vi "LabVIEW.Service.Connect_SNDB_with_API_by_HTTPs_Client.vi"(0 "SN":string="60NJ00143", 1 "VrN":string="I-230032", 4 "Old Product":string="BB0131a-R05", 5 "Changed Product":string="BB0131a-R04", 7 "error in (no error)":errorcluster caption="Fehler (Eingang, kein Fehler)", 8 "Command":T2=enum."Authentication: Creat a token", 9 "Info text":string="\"Test_infoText\"", 12 "Chose Server":string="SNDBTest", 14 "User Update user role\"sn_run_dispach_step\"":bool, 15 "Migrated Vorgang":string="I-250027") -> (10 "Command name":string, 13 "Result_Cluster":T1, 16 "-H":string, 17 "Successful?":bool, 18 "URL":string, 19 "Request body":string, 20 "Body":string, 21 "Test other steps":bool, 24 "Test other steps 2":bool, 25 "Header":string, 27 "error out":errorcluster caption="Fehler (Ausgang)")   [LabVIEW 2026]
uses:
  LabVIEW.Type Definitions/LabVIEW.HTTPs_Client.Command.ctl
  LabVIEW.Type Definitions/LabVIEW.Service.JSON_Input_Command.ctl
  <vilib>/httpClient/ClientHandle.ctl
  <vilib>/JDP Science/JSONtext/Next JSON Value.vi
  <vilib>/JDP Science/JSONtext/String Subset.vi
  <vilib>/JDP Science/JSONtext/support/Strip Quotes and Unescape.vi
  <vilib>/JDP Science/JSONtext/Parsing/Advance past next JSON Value (inlined COPY).vi
  <vilib>/JDP Science/JSONtext/support/Unescape JSON string.vi
  <vilib>/JDP Science/JSONtext/Parsing/Advance past whitespace.vi
  <vilib>/JDP Science/JSONtext/Parsing/Advance past String.vi
  <vilib>/JDP Science/JSONtext/Parsing/Advance past Number.vi
  <vilib>/JDP Science/JSONtext/Parsing/Advance past Line Ending.vi
  <vilib>/JDP Science/JSONtext/support/Format JSON Object.vi
  <vilib>/httpClient/POSTBuffer.vi
  <vilib>/JDP Science/JSONtext/Parsing/Parse Full Path or Item Name.vi
  <vilib>/JDP Science/JSONtext/Parsing/Advance past Array.vi
  <vilib>/JDP Science/JSONtext/Parsing/Advance past Object.vi
  <vilib>/JDP Science/JSONtext/support/Error Cluster From Code.vi
  <vilib>/JDP Science/JSONtext/Offset/Find Item Locations by Path.vi
  <vilib>/httpClient/PUTBuffer.vi
  <vilib>/regexp/Match Regular Expression.xnode
  <vilib>/httpClient/LabVIEWHTTPClient.lvlib
  <vilib>/JDP Science/JSONtext/JSONtext.lvlib
panel:
  out "API Token":string
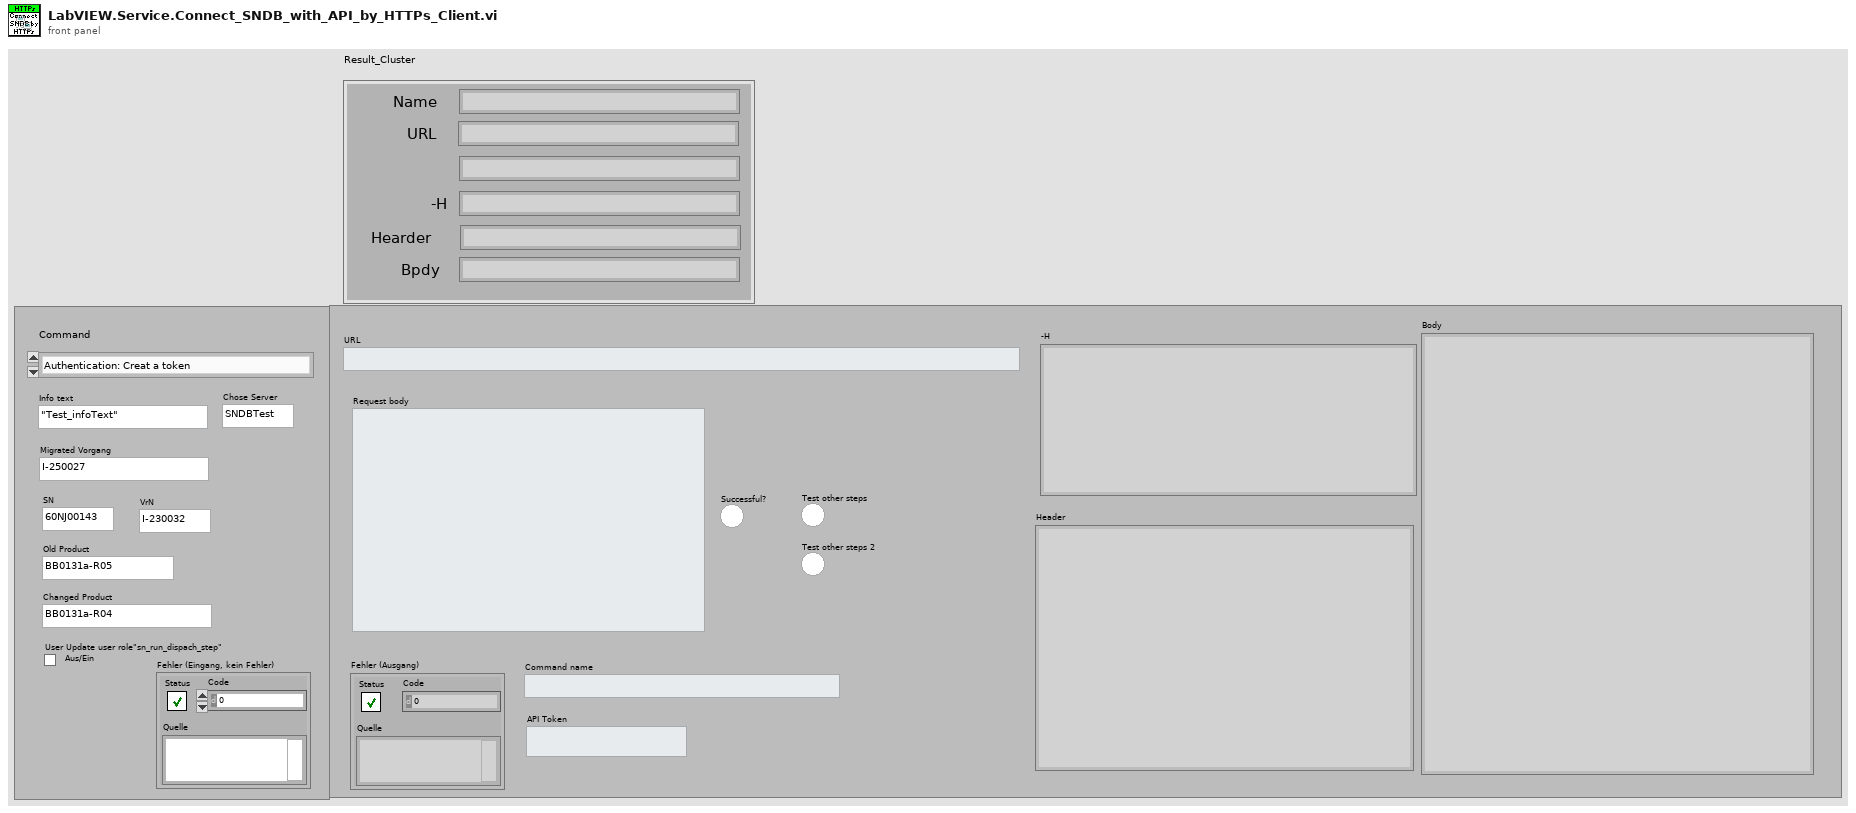
[diagram p1: front panel]
types:
  T1 = cluster{"Name":string, "URL":string, "Request body":string, "-H":string, "Hearder":string, "Bpdy":string}
  T2 = typedef "LabVIEW.HTTPs_Client.Command.ctl" = enum16{"Initialize HTTPS", "Authentication: Creat a token", "Authentication: Get all tokens", "Authentication: Revoke the token", "Label: Creat a label configuration", "Label: Get all configured labels", "Label: Update the label configuration", "Label: Delete the label configuration", "Label: Creat a colour ribbon", "Label: Update the colour ribbon", "Label: Get all colour ribbons", "Label: Delete the colour ribbon", "Label: Creat a label tape", "Label: Update the label tape", "Label: Get all label tapes", "Label: Delete the label tape", "Label: Get all label parameters", "Product: Get all product informations", "Product: Get all reading steps", "Seriennummer: Update the info text", "Seriennummer: Set all step states open", "Seriennummer: Update step states", "Seriennummer: Get data and steps", "Seriennummer: Get all label configurations", "Seriennummer: Create a text report(Prüfbericht)", "Seriennummer: Get the text report(Prüfbericht)", "Seriennummer: Delete the text report(Prüfbericht)", "Seriennummer: Upload a document(txt file)", "Seriennummer: Get the document", "Seriennummer: Get the document thumbnail", "Seriennummer: Delete the document", "Seriennummer: Bulk lookup", "Vorgang: Update the description text", "Vorgang: Migrate serial numbers to a Vorgang", "Vorgang: Migrate serial numbers to a product revision", "Vorgang: Update step states", "Vorgang: Create test reports(Prüfprotokoll)", "Vorgang: Get basic data", "Vorgang: Get serial number data and steps", "Vorgang: Get all serial numbers", "Vorgang: Generate a CSV file", "Vorgang: Generate an XLSX file", "Vorgang: Get a CSV file(Fertigmeldung report)", "Fertigmeldung: Create a Fertigmeldung", "Fertigmeldung: Revert the Fertigmeldung", "User: Get all users", "User: Update an user", "User: Get a single user", "User: Get all user roles", "User: Update a user role", "User: Get a single user role", "User: Get all permissions", "Search: Get Vorgang/Produkt combinations", "Search: Get Vorgang/Produkt/SN combinations", "Search: Get Seriennummern by Vorgang and Produkt", "Search: Lookup Vorgang", "MAC addresses: Get all reserved MAC addresses", "MAC addresses: Get the most recently reserved MAC addresses", "MAC addresses: Get data for a MAC address", "MAC addresses: Reserve MAC addresses for a Seriennummer", "MAC addresses: Mark a reserved MAC address as flashed", "Product: Get possible steps", "Product: Get all products", "Product: Create a new product", "Product: Update a product's data", "Product: Get next product IDs", "Product: Delete a product", "Product properties: Get all product property types", "Search: Find production plan", "Search: Find production plan arrangement", "Health check: Health check", "Deinitialize HTTPs"}
  T3 = typedef "LabVIEW.Service.JSON_Input_Command.ctl" = enum16{"Label configuration", "Label colour ribbon/label tape", "Serial number info text", "Serial number update step", "Serial number bulk lookup", "Vorgang migrate serial numbers to Vorgang", "Vorgang migrate serial numbers to product revision", "Vorgang Update step states", "Fertigmeldung Create/Revert a Fertigmeldung", "User Update a user", "User Update a user role", "Create a new product", "Update a product's data"}
  T4 = cluster{"Name":string, "Value":string, "File":path, "Filename":string, "MIME type":string}
  T5 = enum16{"read csv", "clear csv", "read xlsx", "clear xlsx"}
  T6 = typedef "LabVIEWHTTPClient.lvlib/ClientHandle.ctl" = refnum<k1>
  T7 = cluster{"Name":string, "Value":string, "File":path, "Filename":string, "MIME type":string}[]
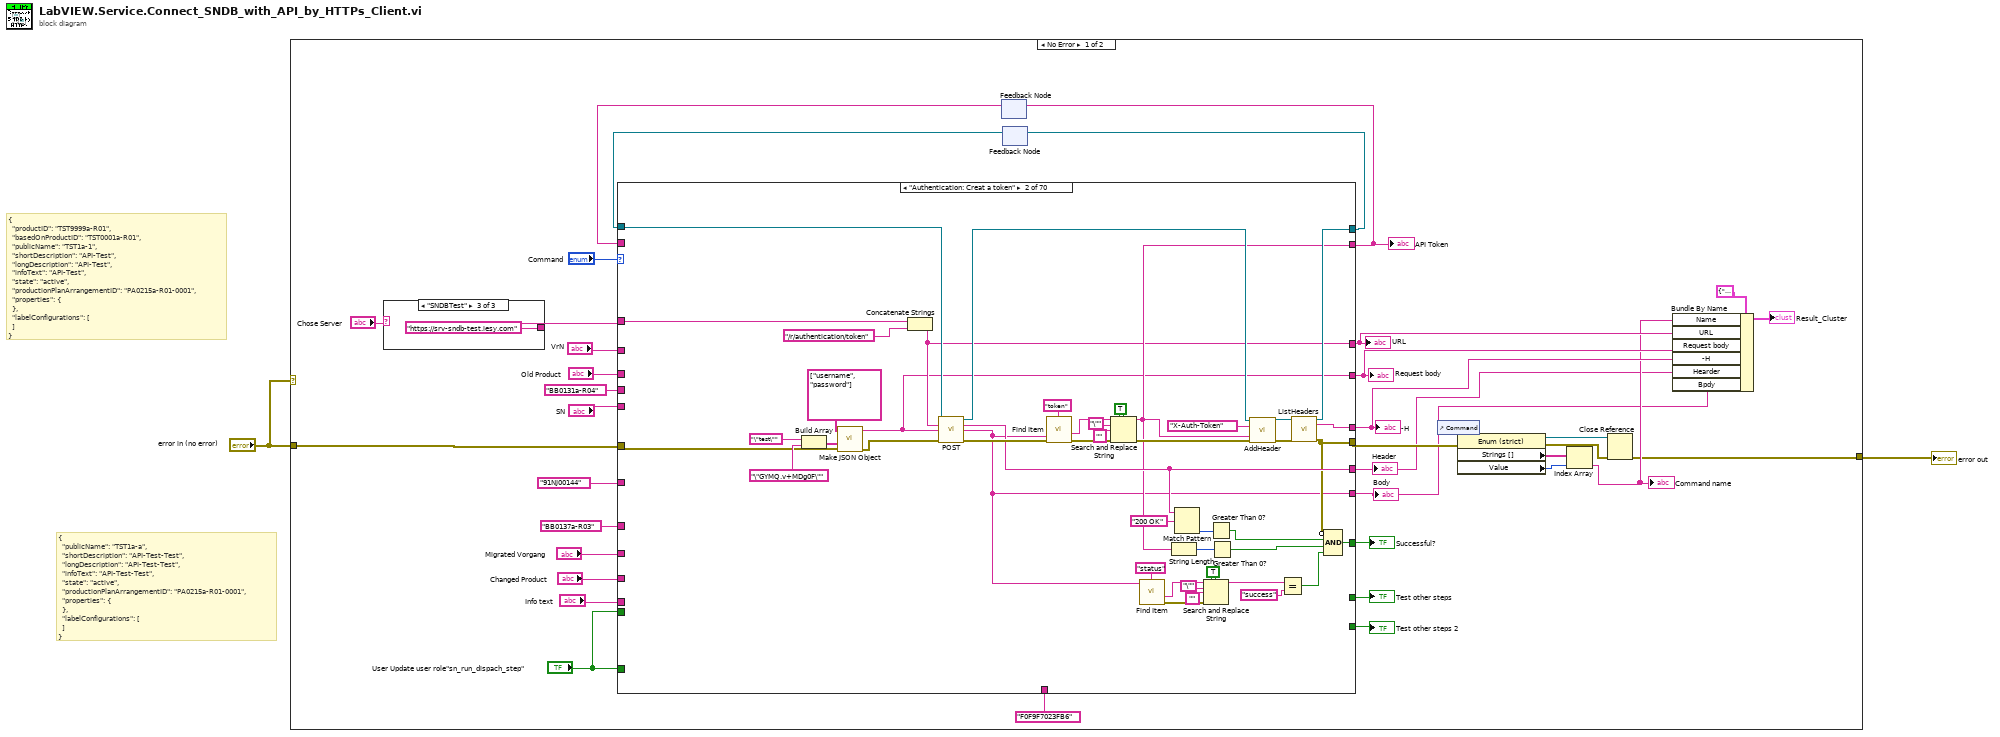
[diagram p0: block diagram]
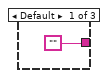
[diagram p2: hidden frame]
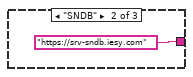
[diagram p3: hidden frame]
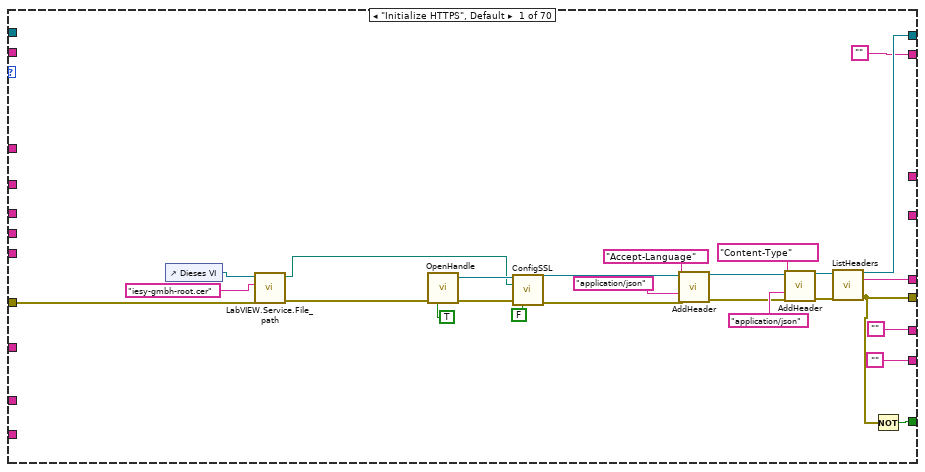
[diagram p4: hidden frame]
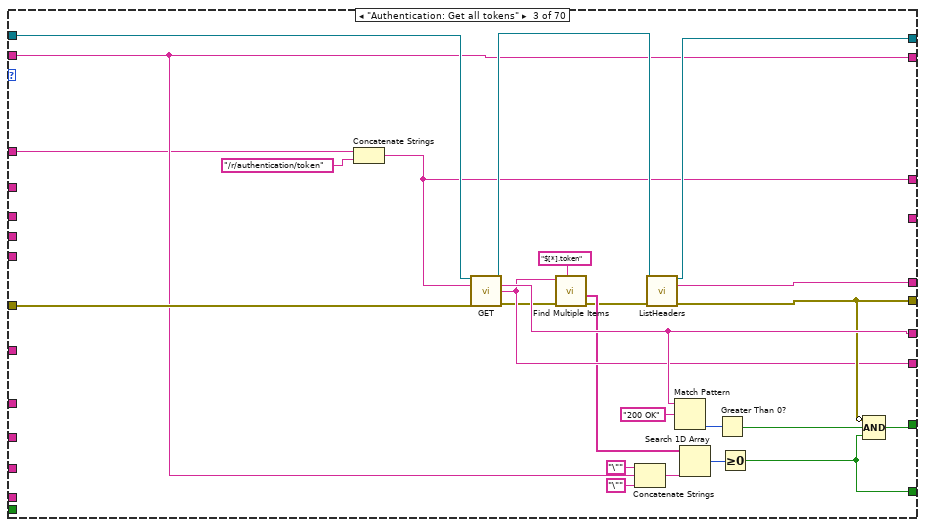
[diagram p5: hidden frame]
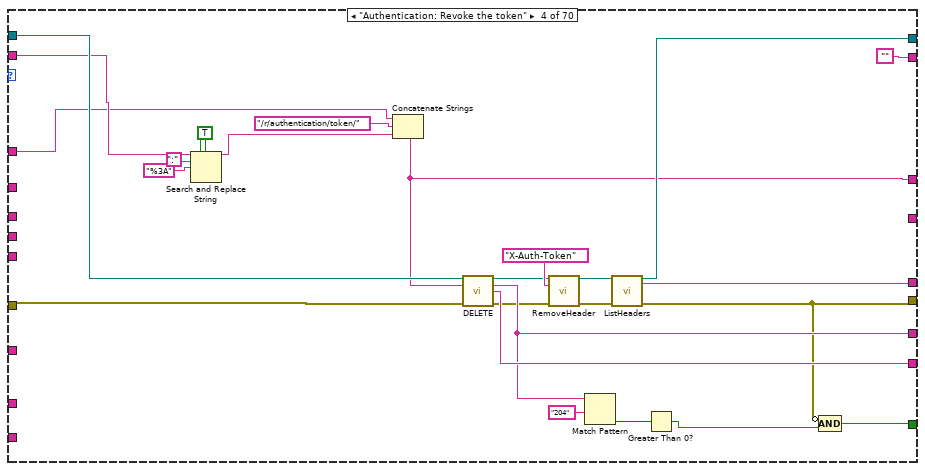
[diagram p6: hidden frame]
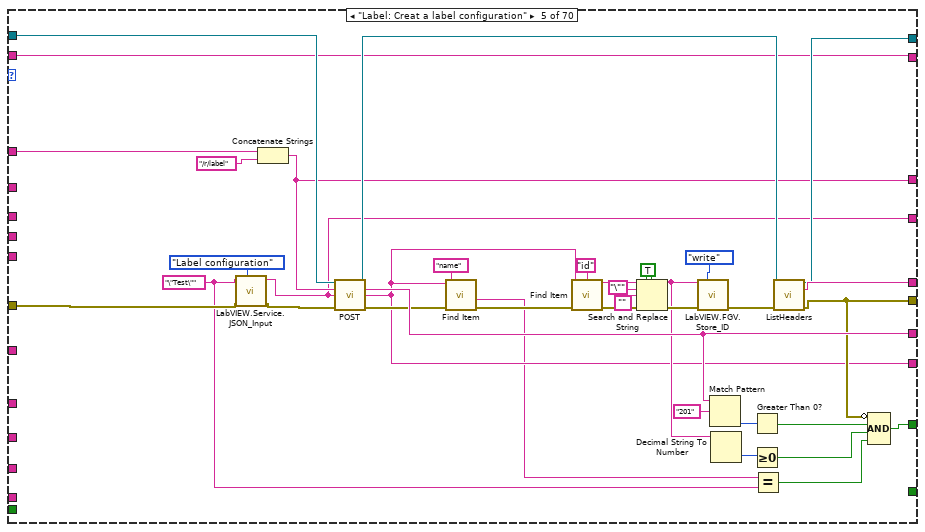
[diagram p7: hidden frame]
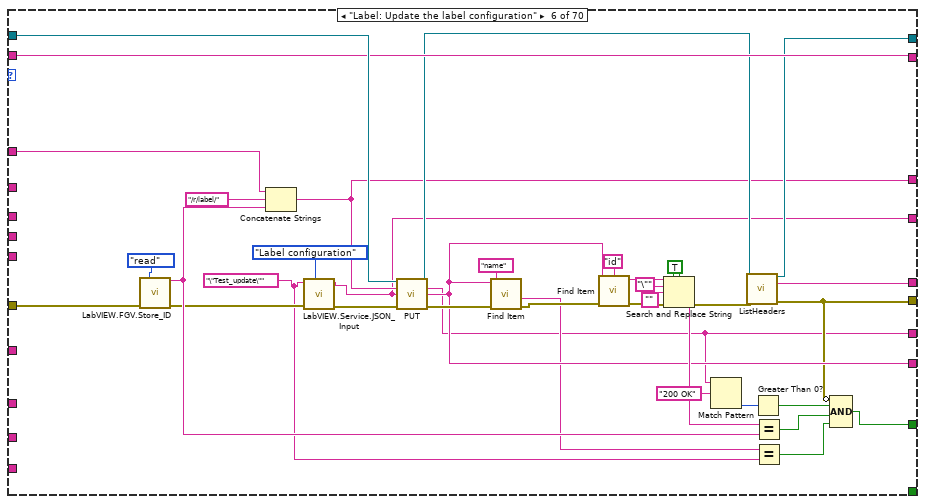
[diagram p8: hidden frame]
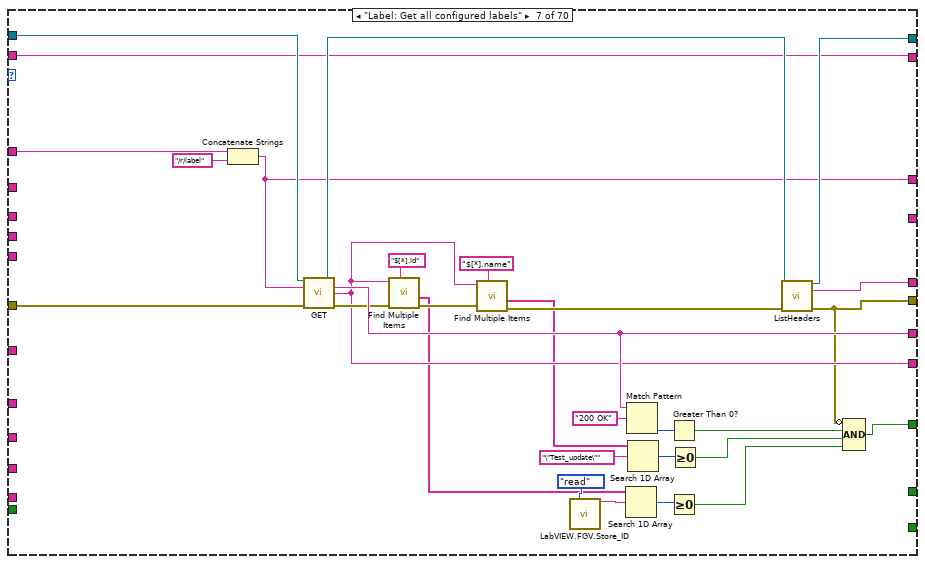
[diagram p9: hidden frame]
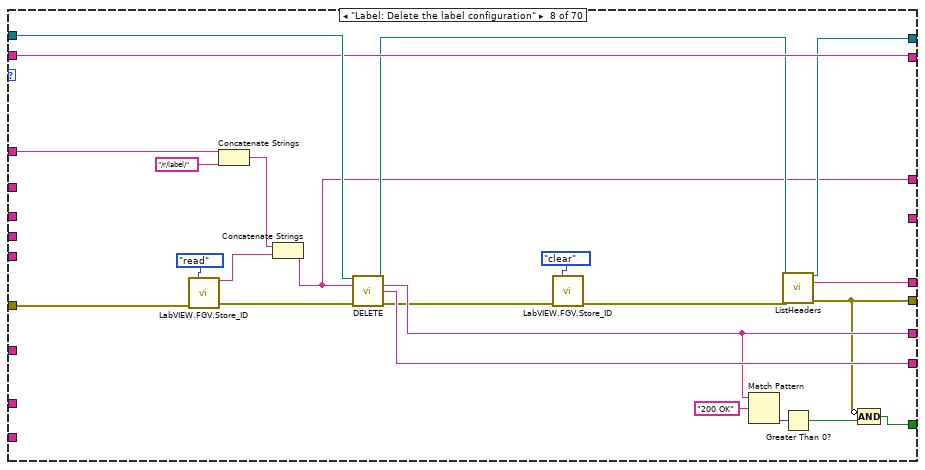
[diagram p10: hidden frame]
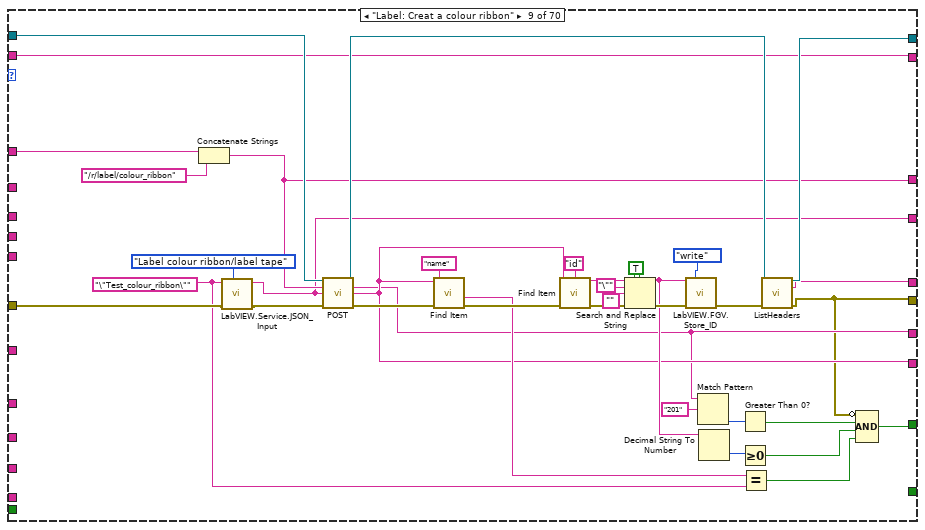
[diagram p11: hidden frame]
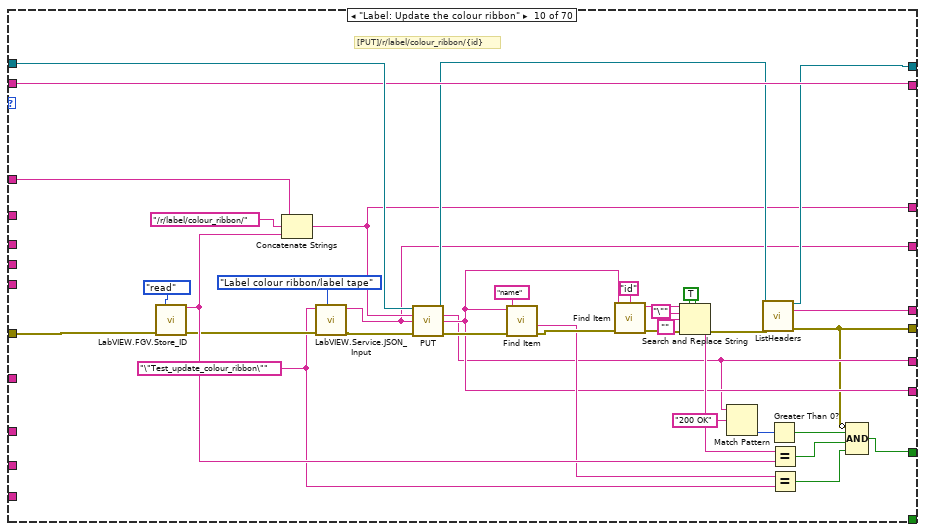
[diagram p12: hidden frame]
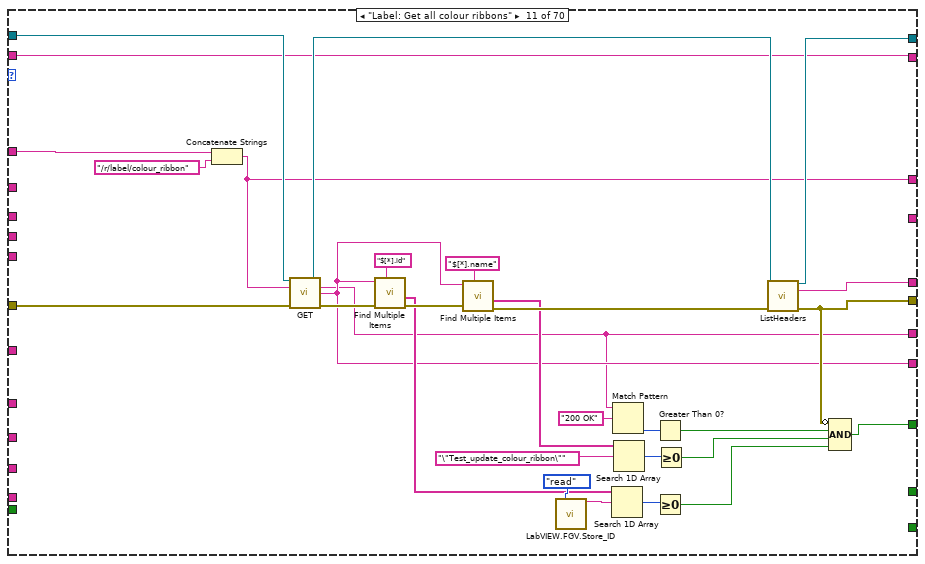
[diagram p13: hidden frame]
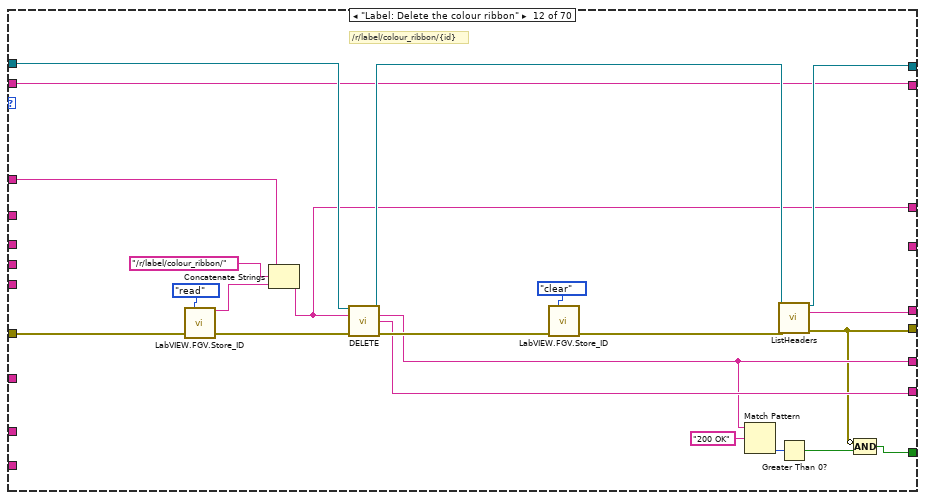
[diagram p14: hidden frame]
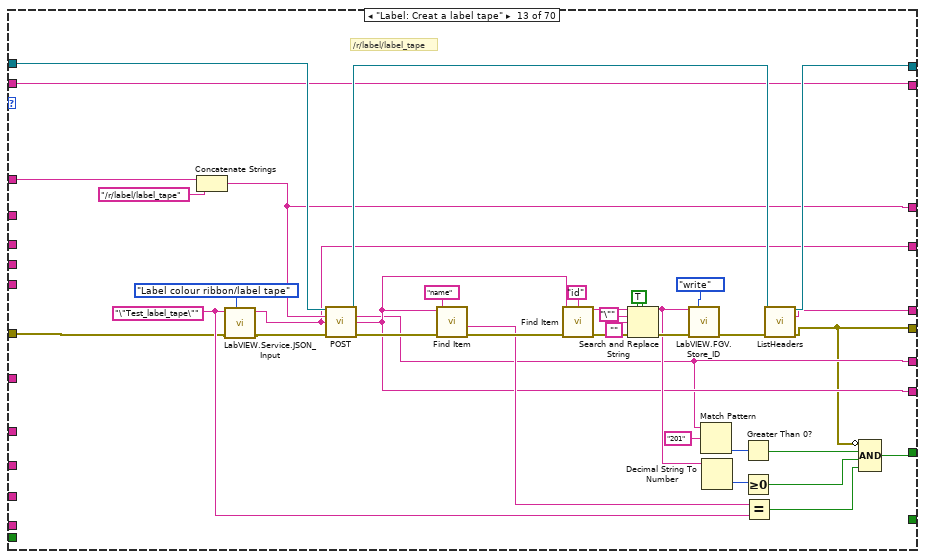
[diagram p15: hidden frame]
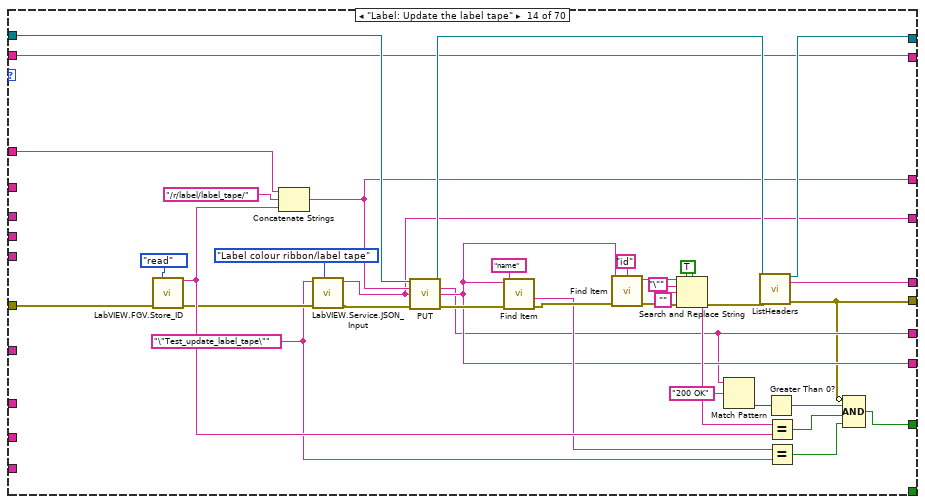
[diagram p16: hidden frame]
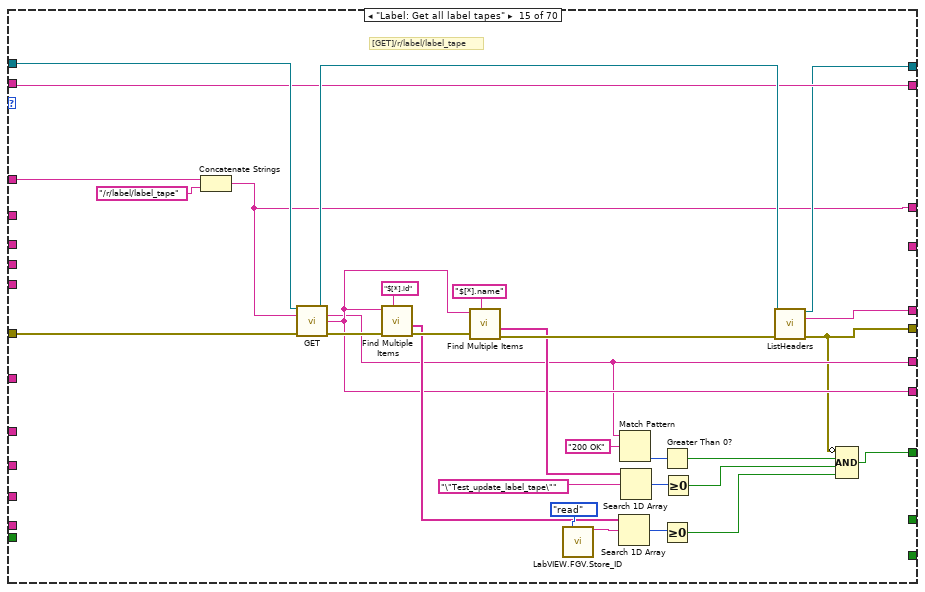
[diagram p17: hidden frame]
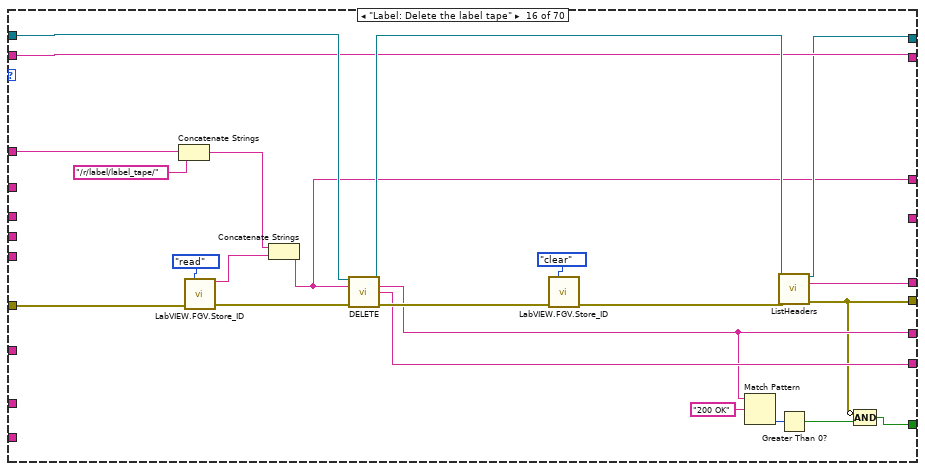
[diagram p18: hidden frame]
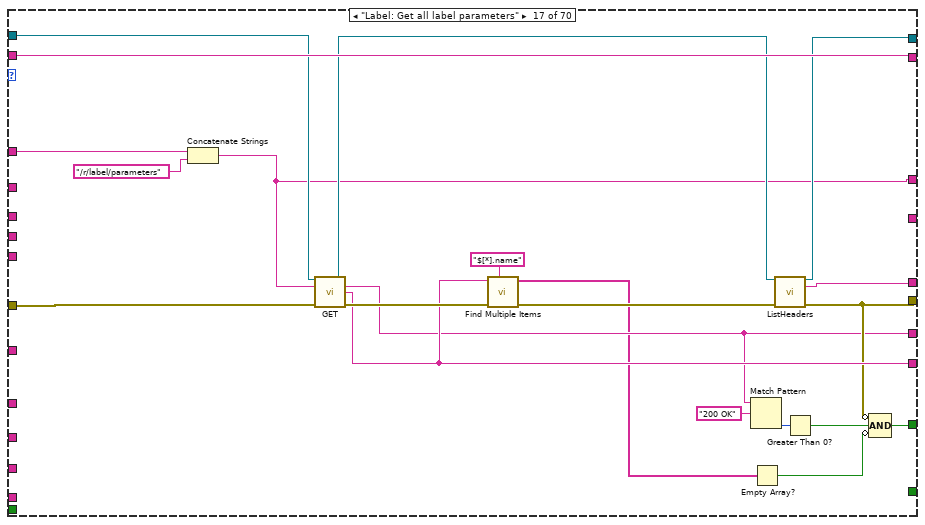
[diagram p19: hidden frame]
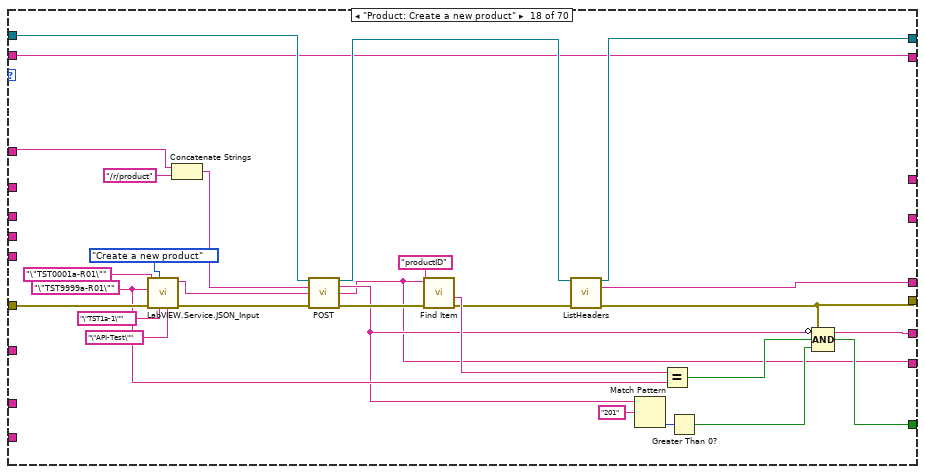
[diagram p20: hidden frame]
diagram:
  # "{\n  \"publicName\": \"TST1a-a\",\n  \"shortDescription\": \"API-Test-Test\",\n  \"longDescription\": \"API-Test-Test\",\n  \"infoText\": \"API-Test-Test\",\n  \"state\": \"active\",\n  \"productionPlanArrangementID\": \"PA0215a-R01-0001\",\n  \"properties\": {\n  },\n  \"labelConfigurations\": [\n  ]\n}"
  # "{\n  \"productID\": \"TST9999a-R01\",\n  \"basedOnProductID\": \"TST0001a-R01\",\n  \"publicName\": \"TST1a-1\",\n  \"shortDescription\": \"API-Test\",\n  \"longDescription\": \"API-Test\",\n  \"infoText\": \"API-Test\",\n  \"state\": \"active\",\n  \"productionPlanArrangementID\": \"PA0215a-R01-0001\",\n  \"properties\": {\n  },\n  \"labelConfigurations\": [ \n  ]\n}"
  n1 = case shown="No Error" "error in (no error)" {
    tunnel: "error in (no error)" -> [w39 w2395]
    tunnel: [w4 w2395] -> w2
    frame No Error {
      n2 = case shown="\"SNDBTest\"" "Chose Server" {
        tunnel: ["" "https://srv-sndb.iesy.com" ("String") "https://srv-sndb-test.iesy.com" ("String")] -> w5
        frame Default {
        }
        frame "SNDB" {
        }
        frame "SNDBTest" {
        }
      }
      n3 = feedback #1() -> (w34:string)  [unwired: 1 in]
      n4 = feedback #2() -> (w36:T6)  [unwired: 1 in]
      n5 = case shown="\"Authentication: Creat a token\"" "Command" {
        tunnel: w39 -> [w43 w97 w137 w157 w170 w233 w266 w285 w296 w343 w376 w402 w425 w461 w498 w529 w563 w583 w612 w640 w670 w685 w712 w728 w756 w781 w800 w837 w895 w963 w1005 w1054 w1085 w1101 w1116 w1190 w1217 w1236 w1286 w1313 w1334 w1370 w1396 w1412 w1468 w1539 w1563 w1600 w1638 w1658 w1701 w1733 w1772 w1797 w1835 w1866 w1892 w1919 w1976 w2021 w2055 w2084 w2111 w2138 w2165 w2194 w2221 w2246 w2267 w2394]
        tunnel: [w56 w92 w133 w159 w198 w214 w263 w282 w300 w336 w369 w397 w421 w457 w494 w525 w558 w566 w605 w638 w650 w682 w701 w733 w753 w778 w789 w825 w885 w959 w996 w1050 w1076 w1092 w1150 w1169 w1199 w1234 w1275 w1304 w1337 w1366 w1403 w1426 w1466 w1528 w1554 w1589 w1627 w1667 w1699 w1731 w1768 w1800 w1824 w1863 w1895 w1923 w1981 w2014 w2048 w2077 w2104 w2131 w2158 w2189 w2216 w2241 w2262 w2391] -> w9
        tunnel: [w53 w94 w134 w160 w196 w213 w264 w283 w304 w330 w372 w403 w427 w463 w499 w530 w559 w587 w606 w641 w665 w686 w713 w732 w757 w776 w795 w826 w886 w965 w998 w1052 w1078 w1102 w1151 w1180 w1207 w1237 w1291 w1305 w1338 w1367 w1404 w1427 w1467 w1529 w1555 w1590 w1628 w1669 w1703 w1735 w1770 w1801 w1831 w1867 w1896 w1924 w1982 w2016 w2050 w2079 w2106 w2133 w2160 w2190 w2217 w2242 w2263 T6 refnum ("client handle out")] -> w37
        tunnel: [w49 w83 w127 w146 w180 w212 w247 w276 w299 w335 w375 w398 w422 w458 w495 w526 w553 w567 w597 w619 w651 w675 w695 w718 w754 w765 w790 w818 w884 w957 w993 w1046 w1072 w1093 w1142 w1175 w1202 w1222 w1260 w1298 w1321 w1351 w1380 w1415 w1458 w1523 w1550 w1584 w1622 w1663 w1680 w1712 w1762 w1788 w1825 w1857 w1884 w1922 w1972 w2011 w2045 w2074 w2101 w2128 w2155 w2183 w2210 w2236 w2257 w2387] -> w14
        tunnel: w36 -> [_ w100 w136 w158 w199 w236 w265 w289 w306 w333 w374 w405 w429 w465 w501 w532 w561 w589 w614 w643 w667 w689 w715 w730 w759 w780 w797 w833 w893 w967 w1004 w1053 w1088 w1104 w1165 w1188 w1215 w1239 w1293 w1311 w1342 w1369 w1407 w1430 w1465 w1538 w1562 w1599 w1637 w1671 w1704 w1736 w1771 w1804 w1834 w1869 w1898 w1928 w1980 w2022 w2056 w2085 w2112 w2139 w2166 w2192 w2219 w2244 w2265 w2390]
        tunnel: ["" w88 w124 "" w195 w235 w242 w288 w303 w332 w367 w396 w426 w462 w500 w531 w562 w586 w608 w631 w664 w681 w693 w729 w750 w763 w794 w832 w892 w964 w1000 w1049 w1077 w1112 w1154 w1179 w1206 w1240 w1290 w1310 w1340 w1372 w1406 w1429 w1463 w1534 w1556 w1598 w1636 w1670 w1700 w1732 w1769 w1802 w1829 w1862 w1900 w1926 w1978 w2015 w2049 w2078 w2105 w2132 w2159 w2193 w2220 w2245 w2266 ""] -> w35
        tunnel: ["" w76 w125 w161 w173 w218 w254 w279 w302 w338 w371 w401 w424 w460 w497 w528 w554 w564 w593 w622 w647 w673 w705 w723 w749 w768 w792 w814 w863 w926 w986 w1017 w1066 w1094 w1124 w1172 w1197 w1228 w1253 w1303 w1331 w1354 w1384 w1419 w1440 w1489 w1547 w1588 w1626 w1652 w1685 w1717 w1742 w1792 w1812 w1848 w1877 w1907 w1955 w2005 w2032 w2064 w2097 w2120 w2147 w2178 w2205 w2230 w2251 w2391] -> w6
        tunnel: ["" w91 w130 w149 w192 w207 w258 w278 w301 w337 w370 w400 w423 w459 w496 w527 w550 w565 w601 w639 w657 w676 w698 w719 w755 w766 w791 w813 w862 w956 w994 w1045 w1073 w1095 w1147 w1176 w1203 w1233 w1272 w1301 w1328 w1353 w1378 w1413 w1457 w1522 w1551 w1582 w1620 w1660 w1679 w1711 w1761 w1787 w1823 w1856 w1885 w1920 w1971 w2013 w2047 w2076 w2103 w2130 w2157 w2184 w2211 w2237 w2258 w2391] -> w7
        tunnel: w34 -> [_ _ w124 w154 w195 w235 w242 w288 w303 w332 w367 w396 w426 w462 w500 w531 w562 w586 w608 w631 w664 w681 w693 w729 w750 w763 w794 w832 w892 w964 w1000 w1049 w1077 w1112 w1154 w1179 w1206 w1240 w1290 w1310 w1340 w1372 w1406 w1429 w1463 w1534 w1556 w1598 w1636 w1670 w1700 w1732 w1769 w1802 w1829 w1862 w1900 w1926 w1978 w2015 w2049 w2078 w2105 w2132 w2159 w2193 w2220 w2245 w2266 _]
        tunnel: [w48 w84 w129 w147 w177 w208 w243 w274 w298 w334 w368 w399 w420 w456 w493 w524 w546 w570 w594 w637 w648 w674 w694 w716 w752 w764 w787 w815 w883 w958 w991 w1018 w1070 w1091 w1139 w1174 w1201 w1220 w1255 w1296 w1320 w1350 w1379 w1414 w1446 w1524 w1548 w1583 w1621 w1662 w1681 w1713 w1758 w1784 w1822 w1858 w1883 w1921 w1970 w2012 w2046 w2075 w2102 w2129 w2156 w2174 w2201 w2234 w2255 w2389] -> w33
        tunnel: w5 -> [_ w72 w116 w139 w166 w202 w239 w270 w293 w329 w366 w395 w419 w455 w491 w523 w545 w590 w616 w628 w663 w688 w710 w726 w746 w779 w801 w831 w891 w962 w1003 w1055 w1087 w1098 w1164 w1185 w1212 w1235 w1289 w1312 w1335 w1371 w1402 w1425 w1462 w1533 w1560 w1596 w1634 w1672 w1678 w1710 w1766 w1799 w1809 w1864 w1894 w1918 w1977 w2020 w2054 w2083 w2110 w2137 w2164 w2188 w2215 w2240 w2261 _]
        tunnel: "Old Product" -> [_ _ _ _ _ _ _ _ _ _ _ _ _ _ _ _ _ _ _ _ _ _ _ _ w736 _ _ _ _ _ _ w1038 _ _ _ _ _ _ w1267 _ _ w1364 w1399 w1422 _ w1531 _ w1592 w1630 _ w1695 w1727 _ _ _ _ _ _ _ _ _ w2071 _ _ _ _ _ _ _ _]
        tunnel: "SN" -> [_ _ _ _ _ _ _ _ _ _ _ _ _ _ _ _ _ _ _ _ _ _ _ _ _ _ w799 w829 w889 w943 _ w1037 w1086 w1097 w1162 w1184 w1211 w1232 w1282 _ w1319 w1359 _ _ _ w1483 w1545 w1573 w1611 w1654 w1693 w1725 _ _ _ _ _ _ _ _ w2033 w2066 _ _ _ w2187 w2214 w2225 _ _]
        tunnel: "VrN" -> [_ _ _ _ _ _ _ _ _ _ _ _ _ _ _ _ _ _ _ _ _ _ _ _ _ _ _ _ _ _ _ w1036 _ _ _ _ _ _ _ w1308 _ w1348 w1401 w1424 w1436 w1532 w1559 w1594 w1632 w1651 w1697 w1729 _ _ _ _ _ _ _ w1998 _ w2073 w2095 _ _ _ _ _ _ _]
        tunnel: "91NJ00144" -> [_ _ _ _ _ _ _ _ _ _ _ _ _ _ _ _ _ _ _ _ _ _ _ _ _ _ _ _ _ _ w990 _ _ _ _ _ _ _ w1280 _ _ _ _ _ _ _ _ _ _ _ _ _ _ _ _ _ _ _ _ _ _ _ _ _ _ _ _ _ _ _]
        tunnel: "BB0137a-R03" -> [_ _ _ _ _ _ _ _ _ _ _ _ _ _ _ _ _ _ _ _ _ _ _ _ _ _ _ _ _ _ _ _ _ _ _ _ _ _ w1265 _ _ _ _ _ _ _ _ _ _ _ _ _ _ _ _ _ _ _ _ _ _ _ _ _ _ _ _ _ _ _]
        tunnel: "Info text" -> [_ _ _ _ _ _ _ _ _ _ _ _ _ _ _ _ _ _ _ _ _ _ _ _ _ _ w786 _ _ w937 _ _ _ _ _ _ _ _ _ w1309 _ _ _ _ w1453 _ _ _ _ _ _ _ _ w1777 w1818 _ _ _ _ _ _ _ _ _ _ _ _ _ _ _]
        tunnel: "Migrated Vorgang" -> [_ _ _ _ _ _ _ _ _ _ _ _ _ _ _ _ _ _ _ _ _ _ _ _ _ _ _ _ _ _ _ _ _ _ _ _ _ _ _ _ w1332 _ _ _ _ _ _ _ _ _ _ _ _ _ _ _ _ _ _ _ _ _ _ _ _ _ _ _ _ _]
        tunnel: "BB0131a-R04" -> [_ _ _ _ _ _ _ _ _ _ _ _ _ _ _ _ _ _ _ _ _ _ _ _ _ _ _ _ _ _ _ _ _ _ _ _ _ _ _ _ _ _ _ _ _ _ _ _ _ _ _ _ _ _ _ _ _ _ _ _ _ _ _ _ _ _ _ _ _ _]
        tunnel: "Changed Product" -> [_ _ _ _ _ _ _ _ _ _ _ _ _ _ _ _ _ _ _ _ _ _ _ _ _ _ _ _ _ _ _ _ _ _ _ _ _ _ _ _ _ w1346 _ _ w1444 _ _ _ _ _ _ _ _ _ _ _ _ _ _ _ _ _ _ _ _ _ _ _ _ _]
        tunnel: "User Update user role\"sn_run_dispach_step\"" -> [_ _ _ _ _ _ _ _ _ _ _ _ _ _ _ _ _ _ _ _ _ _ _ _ _ _ _ _ _ _ _ _ _ _ _ _ _ _ _ _ _ _ _ _ _ _ _ _ _ _ _ _ _ _ _ _ _ w1912 w1956 _ _ _ _ _ _ _ _ _ _ _]
        tunnel: "User Update user role\"sn_run_dispach_step\"" -> [_ _ _ _ _ _ _ _ _ _ _ _ _ _ _ _ _ _ _ _ _ _ _ _ _ _ _ _ _ _ _ _ _ _ _ _ _ _ _ _ _ _ _ _ _ _ _ _ _ _ _ _ _ _ _ _ _ w1911 _ _ _ _ _ _ _ _ _ _ _ _]
        tunnel: [_ _ w114 _ _ _ _ _ _ _ _ _ _ _ _ _ _ _ _ _ _ _ _ _ _ _ _ _ _ w932 _ _ w1059 _ _ _ _ _ _ _ _ _ _ _ w1439 _ w1541 _ _ _ _ _ _ _ w1810 _ _ _ w1954 _ _ w2061 _ _ _ _ _ _ _ _] -> w22
        tunnel: [_ _ _ _ _ _ _ _ _ _ _ _ _ _ _ _ _ _ _ _ _ _ _ _ _ _ _ _ _ w934 _ _ _ _ _ _ _ _ _ _ _ _ _ _ w1438 w1492 _ _ _ _ _ _ _ _ _ _ _ _ _ _ _ _ _ _ _ _ _ _ _ _] -> w21
        tunnel: "F0F9F7023FB6" ("Element") -> [_ _ _ _ _ _ _ _ _ _ _ _ _ _ _ _ _ _ _ _ _ _ _ _ _ _ _ _ _ _ _ _ _ _ _ _ _ _ _ _ _ _ _ _ _ _ _ _ _ _ _ _ _ _ _ _ _ _ _ _ _ _ _ _ _ w2172 w2197 w2224 _ _]
        tunnel: [_ w70 w113 w138 w164 w201 w237 w267 w291 w328 w364 w394 w417 w454 w490 w520 w543 _ _ w627 _ _ _ _ w734 _ w785 w812 w861 w931 w978 w1007 w1067 w1090 w1119 w1168 w1192 w1219 w1250 w1295 w1318 w1345 w1377 w1411 w1432 w1475 w1540 w1571 w1609 w1641 w1676 w1708 w1739 w1775 w1808 w1838 w1870 w1902 w1953 w1992 w2026 w2060 w2089 w2124 w2151 w2170 w2196 w2223 w2254 _] -> w11
        tunnel: [_ w69 _ _ w163 w200 _ _ w290 w327 _ _ w416 w453 _ _ _ _ _ _ _ _ _ _ _ _ w784 w811 w860 _ _ _ _ _ _ _ _ _ w1249 w1294 w1317 w1344 w1376 _ _ _ _ w1565 w1603 _ w1675 w1707 _ w1774 _ _ _ w1901 _ _ _ _ _ _ _ _ _ _ _ _] -> w10
        frame "Initialize HTTPS", Default {
          n6 = control-ref of="Dieses VI"() -> (w47:refnum<vi>)
          n7 = call "LabVIEW.Service.File_path.vi"("Fehler (Eingang, kein Fehler)"=w43, "File name"="iesy-gmbh-root.cer" ("String"), "VI Reference"=w47) -> ("Fehler (Ausgang)"=w44:errorcluster, "Dateipfad-Bedienelement"=w45:path)  [unwired: 7 in]
          n8 = call <vilib>:"OpenHandle.vi"("error in (no error)"=w44, "verify server(true)"=TRUE) -> ("client handle out"=w66:T6, "error out"=w64:errorcluster)  [unwired: 12 in]
          n9 = call <vilib>:"ConfigSSL.vi"("client handle"=w66, "CA certificate file"=w45, "error in (no error)"=w64, "verify server (true)"=FALSE) -> ("client handle out"=w67:T6, "error out"=w65:errorcluster)  [unwired: 10 in]
          n10 = call <vilib>:"AddHeader.vi"("client handle"=w67, "header"="Accept-Language", "value"="application/json", "error in (no error)"=w65) -> ("client handle out"=w60:T6, "error out"=w61:errorcluster)  [unwired: 10 in]
          n11 = call <vilib>:"AddHeader.vi"("client handle"=w60, "header"="Content-Type", "value"="application/json", "error in (no error)"=w61) -> ("client handle out"=w54:T6, "error out"=w55:errorcluster)  [unwired: 10 in]
          n12 = call <vilib>:"ListHeaders.vi"("client handle"=w54, "error in (no error)"=w55) -> ("client handle out"=w53:T6, "headers"=w56:string, "error out"=w49:errorcluster)  [unwired: 11 in]
          n13 = Not(x=w49) -> (.not. x?=w48:bool)
        }
        frame "Authentication: Creat a token" {
          w78 = TRUE ("Alle ersetzen? (F)")
          w105 = TRUE ("Alle ersetzen? (F)")
          n14 = Build Array("\"test\"", "\"GYMQ.v+MDg0F\"") -> (w111:string[])
          n15 = call <vilib>:"Make JSON Object.vi"("error in (no error)"=w97, "JSON Items"=w111, "Item Names"=string[] ["username", "password"]) -> ("error out"=w108:errorcluster, "<JSON>"=w69:string)  [unwired: 7 in]
          n16 = Concatenate Strings(w72, "/r/authentication/token" ("String")) -> (w70:string)
          n17 = call-poly <vilib>:"POST.vi"("client handle"=w100, "url"=w70, "buffer"=w69, "error in (no error)"=w108) -> ("client handle out"=w98:T6, "headers"=w91:string, "body"=w76:string, "error out"=w106:errorcluster)  [unwired: 8 in]
          n18 = call <vilib>:"Find Item.vi"("$Path or Item Name"="token", "error in (no error)"=w106, "JSON"=w76) -> ("error out"=w101:errorcluster, "<JSON>"=w102:string)  [unwired: 5 in, 2 out]
          n19 = Search and Replace String(replace all?=w105, case sensitive?=w105, input string=w102, search string="\"" ("Such-String"), replace string="", error in=w101) -> (result string=w88:string, error out=w96:errorcluster)  [unwired: 2 in, 2 out]
          n20 = call <vilib>:"Find Item.vi"("$Path or Item Name"="status", "JSON"=w76) -> ("error out"=w82:errorcluster, "<JSON>"=w81:string)  [unwired: 6 in, 2 out]
          n21 = String Length(string=w88) -> (length=w87:i32)
          n22 = Match Pattern(string=w91, regular expression="200 OK" ("Regulärer Ausdruck")) -> (offset past match=w89:i32)  [unwired: 1 in, 3 out]
          n23 = Search and Replace String(replace all?=w78, case sensitive?=w78, input string=w81, search string="\"" ("Such-String"), replace string="", error in=w82) -> (result string=w75:string)  [unwired: 2 in, 3 out]
          n24 = Greater Than 0?(x=w89) -> (x > 0?=w86:bool)
          n25 = Greater Than 0?(x=w87) -> (x > 0?=w85:bool)
          n26 = call <vilib>:"AddHeader.vi"("client handle"=w98, "header"="X-Auth-Token", "value"=w88, "error in (no error)"=w96) -> ("client handle out"=w95:T6, "error out"=w93:errorcluster)  [unwired: 10 in]
          n27 = Equal?(x=w75, y="success" ("$Path or Item Name")) -> (x = y?=w73:bool)
          n28 = call <vilib>:"ListHeaders.vi"("client handle"=w95, "error in (no error)"=w93) -> ("client handle out"=w94:T6, "headers"=w92:string, "error out"=w83:errorcluster)  [unwired: 11 in]
          n29 = Compound Arithmetic op=AND ("Mehrfacharithmetik")(invert w83, w86, w85, w73) -> (w84:bool)
        }
        frame "Authentication: Get all tokens" {
          n30 = Concatenate Strings(w116, "/r/authentication/token" ("String")) -> (w113:string)
          n31 = call <vilib>:"GET.vi"("client handle"=w136, "url"=w113, "error in (no error)"=w137) -> ("client handle out"=w135:T6, "headers"=w130:string, "body"=w125:string, "error out"=w118:errorcluster)  [unwired: 9 in]
          n32 = call <vilib>:"Find Multiple Items.vi"("$Path or Item Name"="$[*].token", "error in (no error)"=w118, "JSON"=w125) -> ("error out"=w117:errorcluster, "<JSON>"=w119:string[])  [unwired: 5 in, 2 out]
          n33 = Concatenate Strings("\"" ("String"), w124, "\"" ("String")) -> (w121:string)
          n34 = call <vilib>:"ListHeaders.vi"("client handle"=w135, "error in (no error)"=w117) -> ("client handle out"=w134:T6, "headers"=w133:string, "error out"=w127:errorcluster)  [unwired: 11 in]
          n35 = Match Pattern(string=w130, regular expression="200 OK" ("Regulärer Ausdruck")) -> (offset past match=w131:i32)  [unwired: 1 in, 3 out]
          n36 = Search 1D Array(1D array=w119, element=w121) -> (index of element=w120:i32)  [unwired: 1 in]
          n37 = Greater Than 0?(x=w131) -> (x > 0?=w128:bool)
          n38 = Greater Or Equal To 0?(x=w120) -> (x >= 0?=w114:bool)
          n39 = Compound Arithmetic op=AND ("Mehrfacharithmetik")(invert w127, w128, w114) -> (w129:bool)
        }
        frame "Authentication: Revoke the token" {
          w156 = TRUE ("Alle ersetzen? (F)")
          n40 = Search and Replace String(replace all?=w156, case sensitive?=w156, input string=w154, search string=":" ("Such-String"), replace string="%3A" ("Such-String")) -> (result string=w152:string)  [unwired: 3 in, 3 out]
          n41 = Concatenate Strings(w139, "/r/authentication/token/", w152) -> (w138:string)
          n42 = call <vilib>:"DELETE.vi"("client handle"=w158, "url"=w138, "error in (no error)"=w157) -> ("client handle out"=w140:T6, "headers"=w149:string, "body"=w161:string, "error out"=w143:errorcluster)  [unwired: 9 in]
          n43 = call <vilib>:"RemoveHeader.vi"("client handle"=w140, "header"="X-Auth-Token", "error in (no error)"=w143) -> ("client handle out"=w141:T6, "error out"=w142:errorcluster)  [unwired: 11 in]
          n44 = Match Pattern(string=w149, regular expression="204") -> (offset past match=w151:i32)  [unwired: 1 in, 3 out]
          n45 = call <vilib>:"ListHeaders.vi"("client handle"=w141, "error in (no error)"=w142) -> ("client handle out"=w160:T6, "headers"=w159:string, "error out"=w146:errorcluster)  [unwired: 11 in]
          n46 = Greater Than 0?(x=w151) -> (x > 0?=w148:bool)
          n47 = Compound Arithmetic op=AND ("Mehrfacharithmetik")(invert w146, w148) -> (w147:bool)
        }
        frame "Label: Creat a label configuration" {
          w168 = "\"Test\"" ("Label_Name")
          w190 = TRUE ("Alle ersetzen? (F)")
          n48 = call "LabVIEW.Service.JSON_Input.vi"("Command"=LabVIEW.Service.JSON_Input_Command."Label configuration", "Fehler (Eingang, kein Fehler)"=w170, "Value 2"=w168) -> ("Fehler (Ausgang)"=w169:errorcluster, "<JSON>"=w163:string)  [unwired: 7 in]
          n49 = Concatenate Strings(w166, "/r/label") -> (w164:string)
          n50 = call-poly <vilib>:"POST.vi"("client handle"=w199, "url"=w164, "buffer"=w163, "error in (no error)"=w169) -> ("client handle out"=w197:T6, "headers"=w192:string, "body"=w173:string, "error out"=w175:errorcluster)  [unwired: 8 in]
          n51 = call <vilib>:"Find Item.vi"("$Path or Item Name"="name", "error in (no error)"=w175, "JSON"=w173) -> ("error out"=w174:errorcluster, "<JSON>"=w172:string)  [unwired: 5 in, 2 out]
          n52 = call <vilib>:"Find Item.vi"("$Path or Item Name"="id", "error in (no error)"=w174, "JSON"=w173) -> ("error out"=w186:errorcluster, "<JSON>"=w187:string)  [unwired: 5 in, 2 out]
          n53 = Search and Replace String(replace all?=w190, case sensitive?=w190, input string=w187, search string="\"" ("Such-String"), replace string="", error in=w186) -> (result string=w182:string, error out=w185:errorcluster)  [unwired: 2 in, 2 out]
          n54 = call "LabVIEW.FGV.Store_ID.vi"("ID In"=w182, "Command"=enum16{"clear", "write", "read"}."write", "error in (no error)"=w185) -> ("error out"=w184:errorcluster)  [unwired: 7 in, 5 out]
          n55 = Match Pattern(string=w192, regular expression="201" ("Regulärer Ausdruck")) -> (offset past match=w193:i32)  [unwired: 1 in, 3 out]
          n56 = Decimal String To Number(string=w182) -> (number=w181:i32)  [unwired: 2 in, 1 out]
          n57 = Greater Than 0?(x=w193) -> (x > 0?=w179:bool)
          n58 = Greater Or Equal To 0?(x=w181) -> (x >= 0?=w178:bool)
          n59 = Equal?(x=w172, y=w168) -> (x = y?=w171:bool)
          n60 = call <vilib>:"ListHeaders.vi"("client handle"=w197, "error in (no error)"=w184) -> ("client handle out"=w196:T6, "headers"=w198:string, "error out"=w180:errorcluster)  [unwired: 11 in]
          n61 = Compound Arithmetic op=AND ("Mehrfacharithmetik")(invert w180, w179, w178, w171) -> (w177:bool)
        }
        frame "Label: Update the label configuration" {
          w227 = TRUE ("Alle ersetzen? (F)")
          w204 = "\"Test_update\"" ("Label_Name")
          n62 = call "LabVIEW.FGV.Store_ID.vi"("Command"=enum16{"clear", "write", "read"}."read", "error in (no error)"=w233) -> ("ID Out"=w221:string, "error out"=w206:errorcluster)  [unwired: 8 in, 4 out]
          n63 = Concatenate Strings(w202, "/r/label/", w221) -> (w201:string)
          n64 = call "LabVIEW.Service.JSON_Input.vi"("Command"=LabVIEW.Service.JSON_Input_Command."Label configuration", "Fehler (Eingang, kein Fehler)"=w206, "Value 2"=w204) -> ("Fehler (Ausgang)"=w205:errorcluster, "<JSON>"=w200:string)  [unwired: 7 in]
          n65 = call-poly <vilib>:"PUT.vi"("client handle"=w236, "url"=w201, "buffer"=w200, "error in (no error)"=w205) -> ("client handle out"=w229:T6, "headers"=w207:string, "body"=w218:string, "error out"=w219:errorcluster)  [unwired: 8 in]
          n66 = call <vilib>:"Find Item.vi"("$Path or Item Name"="name", "error in (no error)"=w219, "JSON"=w218) -> ("error out"=w217:errorcluster, "<JSON>"=w216:string)  [unwired: 5 in, 2 out]
          n67 = call <vilib>:"Find Item.vi"("$Path or Item Name"="id", "error in (no error)"=w217, "JSON"=w218) -> ("error out"=w223:errorcluster, "<JSON>"=w224:string)  [unwired: 5 in, 2 out]
          n68 = Search and Replace String(replace all?=w227, case sensitive?=w227, input string=w224, search string="\"" ("Such-String"), replace string="", error in=w223) -> (result string=w222:string, error out=w215:errorcluster)  [unwired: 2 in, 2 out]
          n69 = Match Pattern(string=w207, regular expression="200 OK" ("Regulärer Ausdruck")) -> (offset past match=w230:i32)  [unwired: 1 in, 3 out]
          n70 = call <vilib>:"ListHeaders.vi"("client handle"=w229, "error in (no error)"=w215) -> ("client handle out"=w213:T6, "headers"=w214:string, "error out"=w212:errorcluster)  [unwired: 11 in]
          n71 = Greater Than 0?(x=w230) -> (x > 0?=w211:bool)
          n72 = Equal?(x=w222, y=w221) -> (x = y?=w210:bool)
          n73 = Equal?(x=w216, y=w204) -> (x = y?=w209:bool)
          n74 = Compound Arithmetic op=AND ("Mehrfacharithmetik")(invert w212, w211, w210, w209) -> (w208:bool)
        }
        frame "Label: Get all configured labels" {
          n75 = Concatenate Strings(w239, "/r/label") -> (w237:string)
          n76 = call <vilib>:"GET.vi"("client handle"=w265, "url"=w237, "error in (no error)"=w266) -> ("client handle out"=w262:T6, "headers"=w258:string, "body"=w254:string, "error out"=w256:errorcluster)  [unwired: 9 in]
          n77 = call <vilib>:"Find Multiple Items.vi"("$Path or Item Name"="$[*].id", "error in (no error)"=w256, "JSON"=w254) -> ("error out"=w255:errorcluster, "<JSON>"=w241:string[])  [unwired: 5 in, 2 out]
          n78 = call <vilib>:"Find Multiple Items.vi"("$Path or Item Name"="$[*].name", "error in (no error)"=w255, "JSON"=w254) -> ("error out"=w248:errorcluster, "<JSON>"=w240:string[])  [unwired: 5 in, 2 out]
          n79 = call "LabVIEW.FGV.Store_ID.vi"("Command"=enum16{"clear", "write", "read"}."read") -> ("ID Out"=w252:string)  [unwired: 9 in, 5 out]
          n80 = Search 1D Array(1D array=w241, element=w252) -> (index of element=w251:i32)  [unwired: 1 in]
          n81 = Match Pattern(string=w258, regular expression="200 OK" ("Regulärer Ausdruck")) -> (offset past match=w259:i32)  [unwired: 1 in, 3 out]
          n82 = Search 1D Array(1D array=w240, element="\"Test_update\"") -> (index of element=w249:i32)  [unwired: 1 in]
          n83 = Greater Than 0?(x=w259) -> (x > 0?=w246:bool)
          n84 = Greater Or Equal To 0?(x=w251) -> (x >= 0?=w244:bool)
          n85 = Greater Or Equal To 0?(x=w249) -> (x >= 0?=w245:bool)
          n86 = call <vilib>:"ListHeaders.vi"("client handle"=w262, "error in (no error)"=w248) -> ("client handle out"=w264:T6, "headers"=w263:string, "error out"=w247:errorcluster)  [unwired: 11 in]
          n87 = Compound Arithmetic op=AND ("Mehrfacharithmetik")(invert w247, w246, w245, w244) -> (w243:bool)
        }
        frame "Label: Delete the label configuration" {
          n88 = call "LabVIEW.FGV.Store_ID.vi"("Command"=enum16{"clear", "write", "read"}."read", "error in (no error)"=w285) -> ("ID Out"=w286:string, "error out"=w284:errorcluster)  [unwired: 8 in, 4 out]
          n89 = Concatenate Strings(w270, "/r/label/") -> (w268:string)
          n90 = Concatenate Strings(w268, w286) -> (w267:string)
          n91 = call <vilib>:"DELETE.vi"("client handle"=w289, "url"=w267, "error in (no error)"=w284) -> ("client handle out"=w277:T6, "headers"=w278:string, "body"=w279:string, "error out"=w272:errorcluster)  [unwired: 9 in]
          n92 = call "LabVIEW.FGV.Store_ID.vi"("Command"=enum16{"clear", "write", "read"}."clear", "error in (no error)"=w272) -> ("error out"=w271:errorcluster)  [unwired: 8 in, 5 out]
          n93 = Match Pattern(string=w278, regular expression="200 OK" ("Regulärer Ausdruck")) -> (offset past match=w280:i32)  [unwired: 1 in, 3 out]
          n94 = call <vilib>:"ListHeaders.vi"("client handle"=w277, "error in (no error)"=w271) -> ("client handle out"=w283:T6, "headers"=w282:string, "error out"=w276:errorcluster)  [unwired: 11 in]
          n95 = Greater Than 0?(x=w280) -> (x > 0?=w275:bool)
          n96 = Compound Arithmetic op=AND ("Mehrfacharithmetik")(invert w276, w275) -> (w274:bool)
        }
        frame "Label: Creat a colour ribbon" {
          w294 = "\"Test_colour_ribbon\"" ("Label_Name")
          w323 = TRUE ("Alle ersetzen? (F)")
          n97 = Concatenate Strings(w293, "/r/label/colour_ribbon") -> (w291:string)
          n98 = call "LabVIEW.Service.JSON_Input.vi"("Command"=LabVIEW.Service.JSON_Input_Command."Label colour ribbon/label tape", "Fehler (Eingang, kein Fehler)"=w296, "Value 2"=w294) -> ("Fehler (Ausgang)"=w295:errorcluster, "<JSON>"=w290:string)  [unwired: 7 in]
          n99 = call-poly <vilib>:"POST.vi"("client handle"=w306, "url"=w291, "buffer"=w290, "error in (no error)"=w295) -> ("client handle out"=w305:T6, "headers"=w301:string, "body"=w302:string, "error out"=w310:errorcluster)  [unwired: 8 in]
          n100 = call <vilib>:"Find Item.vi"("$Path or Item Name"="name", "error in (no error)"=w310, "JSON"=w302) -> ("error out"=w309:errorcluster, "<JSON>"=w308:string)  [unwired: 5 in, 2 out]
          n101 = call <vilib>:"Find Item.vi"("$Path or Item Name"="id", "error in (no error)"=w309, "JSON"=w302) -> ("error out"=w319:errorcluster, "<JSON>"=w320:string)  [unwired: 5 in, 2 out]
          n102 = Search and Replace String(replace all?=w323, case sensitive?=w323, input string=w320, search string="\"" ("Such-String"), replace string="", error in=w319) -> (result string=w315:string, error out=w318:errorcluster)  [unwired: 2 in, 2 out]
          n103 = call "LabVIEW.FGV.Store_ID.vi"("ID In"=w315, "Command"=enum16{"clear", "write", "read"}."write", "error in (no error)"=w318) -> ("error out"=w317:errorcluster)  [unwired: 7 in, 5 out]
          n104 = Match Pattern(string=w301, regular expression="201" ("Regulärer Ausdruck")) -> (offset past match=w325:i32)  [unwired: 1 in, 3 out]
          n105 = Decimal String To Number(string=w315) -> (number=w314:i32)  [unwired: 2 in, 1 out]
          n106 = Greater Than 0?(x=w325) -> (x > 0?=w313:bool)
          n107 = Greater Or Equal To 0?(x=w314) -> (x >= 0?=w312:bool)
          n108 = Equal?(x=w308, y=w294) -> (x = y?=w307:bool)
          n109 = call <vilib>:"ListHeaders.vi"("client handle"=w305, "error in (no error)"=w317) -> ("client handle out"=w304:T6, "headers"=w300:string, "error out"=w299:errorcluster)  [unwired: 11 in]
          n110 = Compound Arithmetic op=AND ("Mehrfacharithmetik")(invert w299, w313, w312, w307) -> (w298:bool)
        }
        frame "Label: Update the colour ribbon" {
          w358 = TRUE ("Alle ersetzen? (F)")
          w340 = "\"Test_update_colour_ribbon\"" ("Label_Name")
          # "[PUT]/r/label/colour_ribbon/{id}"
          n111 = call "LabVIEW.FGV.Store_ID.vi"("Command"=enum16{"clear", "write", "read"}."read", "error in (no error)"=w343) -> ("ID Out"=w352:string, "error out"=w342:errorcluster)  [unwired: 8 in, 4 out]
          n112 = Concatenate Strings(w329, "/r/label/colour_ribbon/", w352) -> (w328:string)
          n113 = call "LabVIEW.Service.JSON_Input.vi"("Command"=LabVIEW.Service.JSON_Input_Command."Label colour ribbon/label tape", "Fehler (Eingang, kein Fehler)"=w342, "Value 2"=w340) -> ("Fehler (Ausgang)"=w341:errorcluster, "<JSON>"=w327:string)  [unwired: 7 in]
          n114 = call-poly <vilib>:"PUT.vi"("client handle"=w333, "url"=w328, "buffer"=w327, "error in (no error)"=w341) -> ("client handle out"=w331:T6, "headers"=w337:string, "body"=w338:string, "error out"=w350:errorcluster)  [unwired: 8 in]
          n115 = call <vilib>:"Find Item.vi"("$Path or Item Name"="name", "error in (no error)"=w350, "JSON"=w338) -> ("error out"=w349:errorcluster, "<JSON>"=w348:string)  [unwired: 5 in, 2 out]
          n116 = call <vilib>:"Find Item.vi"("$Path or Item Name"="id", "error in (no error)"=w349, "JSON"=w338) -> ("error out"=w354:errorcluster, "<JSON>"=w355:string)  [unwired: 5 in, 2 out]
          n117 = Search and Replace String(replace all?=w358, case sensitive?=w358, input string=w355, search string="\"" ("Such-String"), replace string="", error in=w354) -> (result string=w353:string, error out=w347:errorcluster)  [unwired: 2 in, 2 out]
          n118 = Match Pattern(string=w337, regular expression="200 OK" ("Regulärer Ausdruck")) -> (offset past match=w360:i32)  [unwired: 1 in, 3 out]
          n119 = call <vilib>:"ListHeaders.vi"("client handle"=w331, "error in (no error)"=w347) -> ("client handle out"=w330:T6, "headers"=w336:string, "error out"=w335:errorcluster)  [unwired: 11 in]
          n120 = Greater Than 0?(x=w360) -> (x > 0?=w346:bool)
          n121 = Equal?(x=w353, y=w352) -> (x = y?=w345:bool)
          n122 = Equal?(x=w348, y=w340) -> (x = y?=w344:bool)
          n123 = Compound Arithmetic op=AND ("Mehrfacharithmetik")(invert w335, w346, w345, w344) -> (w334:bool)
        }
        frame "Label: Get all colour ribbons" {
          n124 = Concatenate Strings(w366, "/r/label/colour_ribbon") -> (w364:string)
          n125 = call <vilib>:"GET.vi"("client handle"=w374, "url"=w364, "error in (no error)"=w376) -> ("client handle out"=w373:T6, "headers"=w370:string, "body"=w371:string, "error out"=w389:errorcluster)  [unwired: 9 in]
          n126 = call <vilib>:"Find Multiple Items.vi"("$Path or Item Name"="$[*].id", "error in (no error)"=w389, "JSON"=w371) -> ("error out"=w388:errorcluster, "<JSON>"=w378:string[])  [unwired: 5 in, 2 out]
          n127 = call <vilib>:"Find Multiple Items.vi"("$Path or Item Name"="$[*].name", "error in (no error)"=w388, "JSON"=w371) -> ("error out"=w382:errorcluster, "<JSON>"=w377:string[])  [unwired: 5 in, 2 out]
          n128 = call "LabVIEW.FGV.Store_ID.vi"("Command"=enum16{"clear", "write", "read"}."read") -> ("ID Out"=w386:string)  [unwired: 9 in, 5 out]
          n129 = Search 1D Array(1D array=w378, element=w386) -> (index of element=w385:i32)  [unwired: 1 in]
          n130 = Match Pattern(string=w370, regular expression="200 OK" ("Regulärer Ausdruck")) -> (offset past match=w391:i32)  [unwired: 1 in, 3 out]
          n131 = Search 1D Array(1D array=w377, element="\"Test_update_colour_ribbon\"") -> (index of element=w383:i32)  [unwired: 1 in]
          n132 = Greater Than 0?(x=w391) -> (x > 0?=w381:bool)
          n133 = Greater Or Equal To 0?(x=w385) -> (x >= 0?=w379:bool)
          n134 = Greater Or Equal To 0?(x=w383) -> (x >= 0?=w380:bool)
          n135 = call <vilib>:"ListHeaders.vi"("client handle"=w373, "error in (no error)"=w382) -> ("client handle out"=w372:T6, "headers"=w369:string, "error out"=w375:errorcluster)  [unwired: 11 in]
          n136 = Compound Arithmetic op=AND ("Mehrfacharithmetik")(invert w375, w381, w380, w379) -> (w368:bool)
        }
        frame "Label: Delete the colour ribbon" {
          # "/r/label/colour_ribbon/{id}"
          n137 = call "LabVIEW.FGV.Store_ID.vi"("Command"=enum16{"clear", "write", "read"}."read", "error in (no error)"=w402) -> ("ID Out"=w413:string, "error out"=w412:errorcluster)  [unwired: 8 in, 4 out]
          n138 = Concatenate Strings(w395, "/r/label/colour_ribbon/", w413) -> (w394:string)
          n139 = call <vilib>:"DELETE.vi"("client handle"=w405, "url"=w394, "error in (no error)"=w412) -> ("client handle out"=w404:T6, "headers"=w400:string, "body"=w401:string, "error out"=w407:errorcluster)  [unwired: 9 in]
          n140 = call "LabVIEW.FGV.Store_ID.vi"("Command"=enum16{"clear", "write", "read"}."clear", "error in (no error)"=w407) -> ("error out"=w406:errorcluster)  [unwired: 8 in, 5 out]
          n141 = Match Pattern(string=w400, regular expression="200 OK" ("Regulärer Ausdruck")) -> (offset past match=w410:i32)  [unwired: 1 in, 3 out]
          n142 = call <vilib>:"ListHeaders.vi"("client handle"=w404, "error in (no error)"=w406) -> ("client handle out"=w403:T6, "headers"=w397:string, "error out"=w398:errorcluster)  [unwired: 11 in]
          n143 = Greater Than 0?(x=w410) -> (x > 0?=w409:bool)
          n144 = Compound Arithmetic op=AND ("Mehrfacharithmetik")(invert w398, w409) -> (w399:bool)
        }
        frame "Label: Creat a label tape" {
          w430 = "\"Test_label_tape\"" ("Label_Name")
          w449 = TRUE ("Alle ersetzen? (F)")
          # "/r/label/label_tape"
          n145 = Concatenate Strings(w419, "/r/label/label_tape") -> (w417:string)
          n146 = call "LabVIEW.Service.JSON_Input.vi"("Command"=LabVIEW.Service.JSON_Input_Command."Label colour ribbon/label tape", "Fehler (Eingang, kein Fehler)"=w425, "Value 2"=w430) -> ("Fehler (Ausgang)"=w431:errorcluster, "<JSON>"=w416:string)  [unwired: 7 in]
          n147 = call-poly <vilib>:"POST.vi"("client handle"=w429, "url"=w417, "buffer"=w416, "error in (no error)"=w431) -> ("client handle out"=w428:T6, "headers"=w423:string, "body"=w424:string, "error out"=w436:errorcluster)  [unwired: 8 in]
          n148 = call <vilib>:"Find Item.vi"("$Path or Item Name"="name", "error in (no error)"=w436, "JSON"=w424) -> ("error out"=w435:errorcluster, "<JSON>"=w434:string)  [unwired: 5 in, 2 out]
          n149 = call <vilib>:"Find Item.vi"("$Path or Item Name"="id", "error in (no error)"=w435, "JSON"=w424) -> ("error out"=w445:errorcluster, "<JSON>"=w446:string)  [unwired: 5 in, 2 out]
          n150 = Search and Replace String(replace all?=w449, case sensitive?=w449, input string=w446, search string="\"" ("Such-String"), replace string="", error in=w445) -> (result string=w441:string, error out=w444:errorcluster)  [unwired: 2 in, 2 out]
          n151 = call "LabVIEW.FGV.Store_ID.vi"("ID In"=w441, "Command"=enum16{"clear", "write", "read"}."write", "error in (no error)"=w444) -> ("error out"=w443:errorcluster)  [unwired: 7 in, 5 out]
          n152 = Match Pattern(string=w423, regular expression="201" ("Regulärer Ausdruck")) -> (offset past match=w451:i32)  [unwired: 1 in, 3 out]
          n153 = Decimal String To Number(string=w441) -> (number=w440:i32)  [unwired: 2 in, 1 out]
          n154 = Greater Than 0?(x=w451) -> (x > 0?=w439:bool)
          n155 = Greater Or Equal To 0?(x=w440) -> (x >= 0?=w438:bool)
          n156 = Equal?(x=w434, y=w430) -> (x = y?=w433:bool)
          n157 = call <vilib>:"ListHeaders.vi"("client handle"=w428, "error in (no error)"=w443) -> ("client handle out"=w427:T6, "headers"=w421:string, "error out"=w422:errorcluster)  [unwired: 11 in]
          n158 = Compound Arithmetic op=AND ("Mehrfacharithmetik")(invert w422, w439, w438, w433) -> (w420:bool)
        }
        frame "Label: Update the label tape" {
          w484 = TRUE ("Alle ersetzen? (F)")
          w467 = "\"Test_update_label_tape\"" ("Label_Name")
          n159 = call "LabVIEW.FGV.Store_ID.vi"("Command"=enum16{"clear", "write", "read"}."read", "error in (no error)"=w461) -> ("ID Out"=w478:string, "error out"=w469:errorcluster)  [unwired: 8 in, 4 out]
          n160 = Concatenate Strings(w455, "/r/label/label_tape/", w478) -> (w454:string)
          n161 = call "LabVIEW.Service.JSON_Input.vi"("Command"=LabVIEW.Service.JSON_Input_Command."Label colour ribbon/label tape", "Fehler (Eingang, kein Fehler)"=w469, "Value 2"=w467) -> ("Fehler (Ausgang)"=w468:errorcluster, "<JSON>"=w453:string)  [unwired: 7 in]
          n162 = call-poly <vilib>:"PUT.vi"("client handle"=w465, "url"=w454, "buffer"=w453, "error in (no error)"=w468) -> ("client handle out"=w464:T6, "headers"=w459:string, "body"=w460:string, "error out"=w476:errorcluster)  [unwired: 8 in]
          n163 = call <vilib>:"Find Item.vi"("$Path or Item Name"="name", "error in (no error)"=w476, "JSON"=w460) -> ("error out"=w475:errorcluster, "<JSON>"=w474:string)  [unwired: 5 in, 2 out]
          n164 = call <vilib>:"Find Item.vi"("$Path or Item Name"="id", "error in (no error)"=w475, "JSON"=w460) -> ("error out"=w480:errorcluster, "<JSON>"=w481:string)  [unwired: 5 in, 2 out]
          n165 = Search and Replace String(replace all?=w484, case sensitive?=w484, input string=w481, search string="\"" ("Such-String"), replace string="", error in=w480) -> (result string=w479:string, error out=w473:errorcluster)  [unwired: 2 in, 2 out]
          n166 = Match Pattern(string=w459, regular expression="200 OK" ("Regulärer Ausdruck")) -> (offset past match=w486:i32)  [unwired: 1 in, 3 out]
          n167 = call <vilib>:"ListHeaders.vi"("client handle"=w464, "error in (no error)"=w473) -> ("client handle out"=w463:T6, "headers"=w457:string, "error out"=w458:errorcluster)  [unwired: 11 in]
          n168 = Greater Than 0?(x=w486) -> (x > 0?=w472:bool)
          n169 = Equal?(x=w479, y=w478) -> (x = y?=w471:bool)
          n170 = Equal?(x=w474, y=w467) -> (x = y?=w470:bool)
          n171 = Compound Arithmetic op=AND ("Mehrfacharithmetik")(invert w458, w472, w471, w470) -> (w456:bool)
        }
        frame "Label: Get all label tapes" {
          # "[GET]/r/label/label_tape"
          n172 = Concatenate Strings(w491, "/r/label/label_tape") -> (w490:string)
          n173 = call <vilib>:"GET.vi"("client handle"=w501, "url"=w490, "error in (no error)"=w498) -> ("client handle out"=w502:T6, "headers"=w496:string, "body"=w497:string, "error out"=w515:errorcluster)  [unwired: 9 in]
          n174 = call <vilib>:"Find Multiple Items.vi"("$Path or Item Name"="$[*].id", "error in (no error)"=w515, "JSON"=w497) -> ("error out"=w514:errorcluster, "<JSON>"=w504:string[])  [unwired: 5 in, 2 out]
          n175 = call <vilib>:"Find Multiple Items.vi"("$Path or Item Name"="$[*].name", "error in (no error)"=w514, "JSON"=w497) -> ("error out"=w508:errorcluster, "<JSON>"=w503:string[])  [unwired: 5 in, 2 out]
          n176 = call "LabVIEW.FGV.Store_ID.vi"("Command"=enum16{"clear", "write", "read"}."read") -> ("ID Out"=w512:string)  [unwired: 9 in, 5 out]
          n177 = Search 1D Array(1D array=w504, element=w512) -> (index of element=w511:i32)  [unwired: 1 in]
          n178 = Match Pattern(string=w496, regular expression="200 OK" ("Regulärer Ausdruck")) -> (offset past match=w517:i32)  [unwired: 1 in, 3 out]
          n179 = Search 1D Array(1D array=w503, element="\"Test_update_label_tape\"") -> (index of element=w509:i32)  [unwired: 1 in]
          n180 = Greater Than 0?(x=w517) -> (x > 0?=w507:bool)
          n181 = Greater Or Equal To 0?(x=w511) -> (x >= 0?=w505:bool)
          n182 = Greater Or Equal To 0?(x=w509) -> (x >= 0?=w506:bool)
          n183 = call <vilib>:"ListHeaders.vi"("client handle"=w502, "error in (no error)"=w508) -> ("client handle out"=w499:T6, "headers"=w494:string, "error out"=w495:errorcluster)  [unwired: 11 in]
          n184 = Compound Arithmetic op=AND ("Mehrfacharithmetik")(invert w495, w507, w506, w505) -> (w493:bool)
        }
        frame "Label: Delete the label tape" {
          n185 = Concatenate Strings(w523, "/r/label/label_tape/") -> (w521:string)
          n186 = call "LabVIEW.FGV.Store_ID.vi"("Command"=enum16{"clear", "write", "read"}."read", "error in (no error)"=w529) -> ("ID Out"=w541:string, "error out"=w540:errorcluster)  [unwired: 8 in, 4 out]
          n187 = Concatenate Strings(w521, w541) -> (w520:string)
          n188 = call <vilib>:"DELETE.vi"("client handle"=w532, "url"=w520, "error in (no error)"=w540) -> ("client handle out"=w533:T6, "headers"=w527:string, "body"=w528:string, "error out"=w535:errorcluster)  [unwired: 9 in]
          n189 = call "LabVIEW.FGV.Store_ID.vi"("Command"=enum16{"clear", "write", "read"}."clear", "error in (no error)"=w535) -> ("error out"=w534:errorcluster)  [unwired: 8 in, 5 out]
          n190 = Match Pattern(string=w527, regular expression="200 OK" ("Regulärer Ausdruck")) -> (offset past match=w538:i32)  [unwired: 1 in, 3 out]
          n191 = call <vilib>:"ListHeaders.vi"("client handle"=w533, "error in (no error)"=w534) -> ("client handle out"=w530:T6, "headers"=w525:string, "error out"=w526:errorcluster)  [unwired: 11 in]
          n192 = Greater Than 0?(x=w538) -> (x > 0?=w537:bool)
          n193 = Compound Arithmetic op=AND ("Mehrfacharithmetik")(invert w526, w537) -> (w524:bool)
        }
        frame "Label: Get all label parameters" {
          n194 = Concatenate Strings(w545, "/r/label/parameters") -> (w543:string)
          n195 = call <vilib>:"GET.vi"("client handle"=w561, "url"=w543, "error in (no error)"=w563) -> ("client handle out"=w560:T6, "headers"=w550:string, "body"=w554:string, "error out"=w556:errorcluster)  [unwired: 9 in]
          n196 = call <vilib>:"Find Multiple Items.vi"("$Path or Item Name"="$[*].name", "error in (no error)"=w556, "JSON"=w554) -> ("error out"=w555:errorcluster, "Item Names"=w548:string[])  [unwired: 5 in, 2 out]
          n197 = Match Pattern(string=w550, regular expression="200 OK" ("Regulärer Ausdruck")) -> (offset past match=w551:i32)  [unwired: 1 in, 3 out]
          n198 = Empty Array?(array=w548) -> (empty?=w547:bool)
          n199 = call <vilib>:"ListHeaders.vi"("client handle"=w560, "error in (no error)"=w555) -> ("client handle out"=w559:T6, "headers"=w558:string, "error out"=w553:errorcluster)  [unwired: 11 in]
          n200 = Greater Than 0?(x=w551) -> (x > 0?=w549:bool)
          n201 = Compound Arithmetic op=AND ("Mehrfacharithmetik")(invert w553, w549, invert w547) -> (w546:bool)
        }
        frame "Product: Create a new product" {
          w572 = "\"TST9999a-R01\"" ("Value 1")
          n202 = call "LabVIEW.Service.JSON_Input.vi"("Value 4"="\"API-Test\"", "Value 3"="\"TST1a-1\"", "Command"=LabVIEW.Service.JSON_Input_Command."Create a new product", "Fehler (Eingang, kein Fehler)"=w583, "Value 1"=w572, "Value 2"="\"TST0001a-R01\"") -> ("Fehler (Ausgang)"=w582:errorcluster, "<JSON>"=w578:string)  [unwired: 4 in]
          n203 = Concatenate Strings(w590, "/r/product" ("String")) -> (w585:string)
          n204 = call-poly <vilib>:"POST.vi"("client handle"=w589, "url"=w585, "buffer"=w578, "error in (no error)"=w582) -> ("client handle out"=w588:T6, "headers"=w565:string, "body"=w564:string, "error out"=w574:errorcluster)  [unwired: 8 in]
          n205 = call <vilib>:"Find Item.vi"("$Path or Item Name"="productID", "error in (no error)"=w574, "JSON"=w564) -> ("error out"=w571:errorcluster, "<JSON>"=w573:string)  [unwired: 5 in, 2 out]
          n206 = call <vilib>:"ListHeaders.vi"("client handle"=w588, "error in (no error)"=w571) -> ("client handle out"=w587:T6, "headers"=w566:string, "error out"=w567:errorcluster)  [unwired: 11 in]
          n207 = Match Pattern(string=w565, regular expression="201" ("Regulärer Ausdruck")) -> (offset past match=w576:i32)  [unwired: 1 in, 3 out]
          n208 = Equal?(x=w573, y=w572) -> (x = y?=w569:bool)
          n209 = Greater Than 0?(x=w576) -> (x > 0?=w568:bool)
          n210 = Compound Arithmetic op=AND ("Mehrfacharithmetik")(invert w567, w569, w568) -> (w570:bool)
        }
        frame "Product: Update a product's data" {
          w598 = "\"API-Test-Test\"" ("Value 1")
          n211 = call "LabVIEW.Service.JSON_Input.vi"("Command"=LabVIEW.Service.JSON_Input_Command."Update a product's data", "Fehler (Eingang, kein Fehler)"=w612, "Value 1"=w598) -> ("Fehler (Ausgang)"=w611:errorcluster, "<JSON>"=w610:string)  [unwired: 7 in]
          n212 = Concatenate Strings(w616, "/r/product/" ("String"), "TST9999a-R01" ("String")) -> (w609:string)
          n213 = call-poly <vilib>:"PUT.vi"("client handle"=w614, "url"=w609, "buffer"=w610, "error in (no error)"=w611) -> ("client handle out"=w607:T6, "headers"=w601:string, "body"=w593:string, "error out"=w600:errorcluster)  [unwired: 8 in]
          n214 = call <vilib>:"Find Item.vi"("$Path or Item Name"="shortDescription", "error in (no error)"=w600, "JSON"=w593) -> ("error out"=w592:errorcluster, "<JSON>"=w599:string)  [unwired: 5 in, 2 out]
          n215 = Match Pattern(string=w601, regular expression="200" ("Regulärer Ausdruck")) -> (offset past match=w603:i32)  [unwired: 1 in, 3 out]
          n216 = Equal?(x=w599, y=w598) -> (x = y?=w596:bool)
          n217 = Greater Than 0?(x=w603) -> (x > 0?=w595:bool)
          n218 = call <vilib>:"ListHeaders.vi"("client handle"=w607, "error in (no error)"=w592) -> ("client handle out"=w606:T6, "headers"=w605:string, "error out"=w597:errorcluster)  [unwired: 11 in]
          n219 = Compound Arithmetic op=AND ("Mehrfacharithmetik")(invert w597, w596, w595) -> (w594:bool)
        }
        frame "Product: Get all product informations" {
          w626 = "TST9999a-R01"
          w630 = "\"" ("String")
          # "/r/product/{productName}"
          n220 = Concatenate Strings(w628, "/r/product/", w626) -> (w627:string)
          n221 = call <vilib>:"GET.vi"("client handle"=w643, "url"=w627, "error in (no error)"=w640) -> ("client handle out"=w642:T6, "headers"=w639:string, "body"=w622:string, "error out"=w634:errorcluster)  [unwired: 9 in]
          n222 = call <vilib>:"Find Item.vi"("$Path or Item Name"="productID", "error in (no error)"=w634, "JSON"=w622) -> ("error out"=w624:errorcluster, "<JSON>"=w633:string)  [unwired: 5 in, 2 out]
          n223 = call <vilib>:"Find Item.vi"("$Path or Item Name"="shortDescription", "error in (no error)"=w624, "JSON"=w622) -> ("error out"=w623:errorcluster, "<JSON>"=w620:string)  [unwired: 5 in, 2 out]
          n224 = Match Pattern(string=w639, regular expression="200" ("Regulärer Ausdruck")) -> (offset past match=w645:i32)  [unwired: 1 in, 3 out]
          n225 = Concatenate Strings(w630, w626, w630) -> (w629:string)
          n226 = Equal?(x=w633, y=w629) -> (x = y?=w632:bool)
          n227 = Greater Than 0?(x=w645) -> (x > 0?=w644:bool)
          n228 = Equal?(x=w620, y="\"API-Test-Test\"" ("Value 1")) -> (x = y?=w618:bool)
          n229 = call <vilib>:"ListHeaders.vi"("client handle"=w642, "error in (no error)"=w623) -> ("client handle out"=w641:T6, "headers"=w638:string, "error out"=w619:errorcluster)  [unwired: 11 in]
          n230 = Compound Arithmetic op=AND ("Mehrfacharithmetik")(invert w619, w618, w644, w632) -> (w637:bool)
        }
        frame "Product: Get next product IDs" {
          n231 = Concatenate Strings(w663, "/r/product/", "TST9999a-R01", "/next_available_ids" ("String")) -> (w661:string)
          n232 = call <vilib>:"GET.vi"("client handle"=w667, "url"=w661, "error in (no error)"=w670) -> ("client handle out"=w666:T6, "headers"=w657:string, "body"=w647:string, "error out"=w655:errorcluster)  [unwired: 9 in]
          n233 = call <vilib>:"Find Item.vi"("$Path or Item Name"="nextProductVariant", "error in (no error)"=w655, "JSON"=w647) -> ("error out"=w652:errorcluster, "<JSON>"=w649:string)  [unwired: 5 in, 2 out]
          n234 = Equal?(x=w649, y="\"TST9999b-R01\"") -> (x = y?=w654:bool)
          n235 = Match Pattern(string=w657, regular expression="200" ("Regulärer Ausdruck")) -> (offset past match=w659:i32)  [unwired: 1 in, 3 out]
          n236 = Greater Than 0?(x=w659) -> (x > 0?=w658:bool)
          n237 = call <vilib>:"ListHeaders.vi"("client handle"=w666, "error in (no error)"=w652) -> ("client handle out"=w665:T6, "headers"=w650:string, "error out"=w651:errorcluster)  [unwired: 11 in]
          n238 = Compound Arithmetic op=AND ("Mehrfacharithmetik")(invert w651, w654, w658) -> (w648:bool)
        }
        frame "Product: Get possible steps" {
          n239 = Concatenate Strings(w688, "/r/product/", "possible_steps") -> (w690:string)
          n240 = call <vilib>:"GET.vi"("client handle"=w689, "url"=w690, "error in (no error)"=w685) -> ("client handle out"=w687:T6, "headers"=w676:string, "body"=w673:string, "error out"=w683:errorcluster)  [unwired: 9 in]
          n241 = call <vilib>:"Find Multiple Items.vi"("$Path or Item Name"="$[*].id", "error in (no error)"=w683, "JSON"=w673) -> ("error out"=w680:errorcluster, "<JSON>"=w672:string[])  [unwired: 5 in, 2 out]
          n242 = Empty Array?(array=w672) -> (empty?=w671:bool)
          n243 = Match Pattern(string=w676, regular expression="200" ("Regulärer Ausdruck")) -> (offset past match=w678:i32)  [unwired: 1 in, 3 out]
          n244 = call <vilib>:"ListHeaders.vi"("client handle"=w687, "error in (no error)"=w680) -> ("client handle out"=w686:T6, "headers"=w682:string, "error out"=w675:errorcluster)  [unwired: 11 in]
          n245 = Greater Than 0?(x=w678) -> (x > 0?=w677:bool)
          n246 = Compound Arithmetic op=AND ("Mehrfacharithmetik")(invert w675, invert w671, w677) -> (w674:bool)
        }
        frame "Product: Get all products" {
          n247 = Concatenate Strings(w710, "/r/product") -> (w709:string)
          n248 = call <vilib>:"GET.vi"("client handle"=w715, "url"=w709, "error in (no error)"=w712) -> ("client handle out"=w714:T6, "headers"=w698:string, "body"=w705:string, "error out"=w707:errorcluster)  [unwired: 9 in]
          n249 = call <vilib>:"Find Multiple Items.vi"("$Path or Item Name"="$[*].productID", "error in (no error)"=w707, "JSON"=w705) -> ("error out"=w706:errorcluster, "<JSON>"=w704:string[])  [unwired: 5 in, 2 out]
          n250 = Search 1D Array(1D array=w704, element="\"TST9999a-R01\"" ("y")) -> (index of element=w702:i32)  [unwired: 1 in]
          n251 = Match Pattern(string=w698, regular expression="200" ("Regulärer Ausdruck")) -> (offset past match=w699:i32)  [unwired: 1 in, 3 out]
          n252 = Greater Than 0?(x=w699) -> (x > 0?=w697:bool)
          n253 = Greater Or Equal To 0?(x=w702) -> (x >= 0?=w696:bool)
          n254 = call <vilib>:"ListHeaders.vi"("client handle"=w714, "error in (no error)"=w706) -> ("client handle out"=w713:T6, "headers"=w701:string, "error out"=w695:errorcluster)  [unwired: 11 in]
          n255 = Compound Arithmetic op=AND ("Mehrfacharithmetik")(invert w695, w696, w697) -> (w694:bool)
        }
        frame "Product: Delete a product" {
          n256 = Concatenate Strings(w726, "/r/product/", "TST9999a-R01") -> (w724:string)
          n257 = call <vilib>:"DELETE.vi"("client handle"=w730, "url"=w724, "error in (no error)"=w728) -> ("client handle out"=w731:T6, "headers"=w719:string, "body"=w723:string, "error out"=w722:errorcluster)  [unwired: 9 in]
          n258 = Match Pattern(string=w719, regular expression="204" ("Regulärer Ausdruck")) -> (offset past match=w720:i32)  [unwired: 1 in, 3 out]
          n259 = Greater Than 0?(x=w720) -> (x > 0?=w717:bool)
          n260 = call <vilib>:"ListHeaders.vi"("client handle"=w731, "error in (no error)"=w722) -> ("client handle out"=w732:T6, "headers"=w733:string, "error out"=w718:errorcluster)  [unwired: 11 in]
          n261 = Compound Arithmetic op=AND ("Mehrfacharithmetik")(invert w718, w717) -> (w716:bool)
        }
        frame "Product: Get all reading steps" {
          n262 = Concatenate Strings(w746, "/r/revision/", w736, "/einleseschritte" ("String")) -> (w734:string)
          n263 = call <vilib>:"GET.vi"("client handle"=w759, "url"=w734, "error in (no error)"=w756) -> ("client handle out"=w758:T6, "headers"=w755:string, "body"=w749:string, "error out"=w743:errorcluster)  [unwired: 9 in]
          n264 = call <vilib>:"Find Multiple Items.vi"("$Path or Item Name"="$[*].id", "error in (no error)"=w743, "JSON"=w749) -> ("error out"=w747:errorcluster, "<JSON>"=w741:string[])  [unwired: 5 in, 2 out]
          n265 = Index Array(array=w741, index=0 ("Index")) -> (element=w739:string)
          n266 = call "LabVIEW.FGV.Store_ID.vi"("Command"=enum16{"clear", "write", "read"}."read", "error in (no error)"=w747) -> ("Step IDs out[]"=w742:string[], "error out"=w735:errorcluster)  [unwired: 8 in, 4 out]
          n267 = Search 1D Array(1D array=w742, element=w739) -> (index of element=w738:i32)  [unwired: 1 in]
          n268 = Match Pattern(string=w755, regular expression="200 OK" ("Regulärer Ausdruck")) -> (offset past match=w761:i32)  [unwired: 1 in, 3 out]
          n269 = Greater Or Equal To 0?(x=w738) -> (x >= 0?=w737:bool)
          n270 = Greater Than 0?(x=w761) -> (x > 0?=w760:bool)
          n271 = call <vilib>:"ListHeaders.vi"("client handle"=w758, "error in (no error)"=w735) -> ("client handle out"=w757:T6, "headers"=w753:string, "error out"=w754:errorcluster)  [unwired: 11 in]
          n272 = Compound Arithmetic op=AND ("Mehrfacharithmetik")(invert w754, w760, w737) -> (w752:bool)
        }
        frame "Product properties: Get all product property types" {
          n273 = Concatenate Strings(w779, "/r/product_property") -> (w782:string)
          n274 = call <vilib>:"GET.vi"("client handle"=w780, "url"=w782, "error in (no error)"=w781) -> ("client handle out"=w777:T6, "headers"=w766:string, "body"=w768:string, "error out"=w770:errorcluster)  [unwired: 9 in]
          n275 = call <vilib>:"Find Multiple Items.vi"("$Path or Item Name"="$[*].id", "error in (no error)"=w770, "JSON"=w768) -> ("error out"=w769:errorcluster, "<JSON>"=w767:string[])  [unwired: 5 in, 2 out]
          n276 = Empty Array?(array=w767) -> (empty?=w771:bool)
          n277 = Match Pattern(string=w766, regular expression="200" ("Regulärer Ausdruck")) -> (offset past match=w773:i32)  [unwired: 1 in, 3 out]
          n278 = Greater Than 0?(x=w773) -> (x > 0?=w772:bool)
          n279 = call <vilib>:"ListHeaders.vi"("client handle"=w777, "error in (no error)"=w769) -> ("client handle out"=w776:T6, "headers"=w778:string, "error out"=w765:errorcluster)  [unwired: 11 in]
          n280 = Compound Arithmetic op=AND ("Mehrfacharithmetik")(invert w765, invert w771, w772) -> (w764:bool)
        }
        frame "Seriennummer: Update the info text" {
          # "/r/seriennummer/{seriennummer}/infotext"
          n281 = Concatenate Strings(w801, "/r/seriennummer/", w799, "/infotext" ("String")) -> (w785:string)
          n282 = call "LabVIEW.Service.JSON_Input.vi"("Command"=LabVIEW.Service.JSON_Input_Command."Serial number info text", "Fehler (Eingang, kein Fehler)"=w800, "Value 1"=w786) -> ("Fehler (Ausgang)"=w803:errorcluster, "<JSON>"=w784:string)  [unwired: 7 in]
          n283 = call-poly <vilib>:"PUT.vi"("client handle"=w797, "url"=w785, "buffer"=w784, "error in (no error)"=w803) -> ("client handle out"=w796:T6, "headers"=w791:string, "body"=w792:string, "error out"=w806:errorcluster)  [unwired: 8 in]
          n284 = call <vilib>:"Find Item.vi"("$Path or Item Name"="infoText", "error in (no error)"=w806, "JSON"=w792) -> ("error out"=w793:errorcluster, "<JSON>"=w805:string)  [unwired: 5 in, 2 out]
          n285 = Match Pattern(string=w791, regular expression="200 OK" ("Regulärer Ausdruck")) -> (offset past match=w808:i32)  [unwired: 1 in, 3 out]
          n286 = call <vilib>:"ListHeaders.vi"("client handle"=w796, "error in (no error)"=w793) -> ("client handle out"=w795:T6, "headers"=w789:string, "error out"=w790:errorcluster)  [unwired: 11 in]
          n287 = Greater Than 0?(x=w808) -> (x > 0?=w804:bool)
          n288 = Equal?(x=w805, y=w786) -> (x = y?=w788:bool)
          n289 = Compound Arithmetic op=AND ("Mehrfacharithmetik")(invert w790, w804, w788) -> (w787:bool)
        }
        frame "Seriennummer: Set all step states open" {
          # "/r/seriennummer/{seriennummer}/update_step"
          n290 = call "LabVIEW.FGV.Store_ID.vi"("Command"=enum16{"clear", "write", "read"}."read", "error in (no error)"=w837) -> ("Step IDs out[]"=w834:string[], "Step types out[]"=w835:string[], "error out"=w836:errorcluster)  [unwired: 8 in, 3 out]
          n291 = Concatenate Strings(w831, "/r/seriennummer/" ("String"), w829, "/update_step" ("String")) -> (w812:string)
          n292 = for {
            tunnel: w835 -> [w857] mode=indexing
            tunnel: w834 -> [w856] mode=indexing
            shift-right: [w851] -> w827
            shift-left: w833 -> [w852]
            shift-right: [w850] -> w823
            shift-left: w836 -> [w859]
            tunnel: w812 -> [w849]
            tunnel: [w845] -> w821 mode=indexing
            tunnel: [w844] -> w814
            tunnel: [w843] -> w813
            tunnel: [w842] -> w811
            n293 = Build Array(w857, w856, "\"open\"" ("Element"), "\"\"" ("Element")) -> (w854:string[])
            n294 = call "LabVIEW.Service.JSON_Input.vi"("Command"=LabVIEW.Service.JSON_Input_Command."Serial number update step", "Fehler (Eingang, kein Fehler)"=w859, "Value[]"=w854) -> ("Fehler (Ausgang)"=w853:errorcluster, "<JSON>"=w842:string)  [unwired: 7 in]
            n295 = call-poly <vilib>:"POST.vi"("client handle"=w852, "url"=w849, "buffer"=w842, "error in (no error)"=w853) -> ("client handle out"=w851:T6, "headers"=w843:string, "body"=w844:string, "error out"=w850:errorcluster)  [unwired: 8 in]
            n296 = Match Pattern(string=w843, regular expression="200 OK" ("Regulärer Ausdruck")) -> (offset past match=w846:i32)  [unwired: 1 in, 3 out]
            n297 = Greater Than 0?(x=w846) -> (x > 0?=w845:bool)
          }
          n298 = And Array Elements(Boolean array=w821) -> (logical AND=w816:bool)
          n299 = call <vilib>:"Find Multiple Items.vi"("$Path or Item Name"="$.steps[*].state", "error in (no error)"=w823, "JSON"=w814) -> ("error out"=w820:errorcluster, "<JSON>"=w822:string[])  [unwired: 5 in, 2 out]
          n300 = for {
            tunnel: w822 -> [w841] mode=indexing
            tunnel: [w839] -> w819 mode=indexing
            n301 = Equal?(x=w841, y="\"open\"" ("Element")) -> (x = y?=w839:bool)
          }
          n302 = And Array Elements(Boolean array=w819) -> (logical AND=w817:bool)
          n303 = call <vilib>:"ListHeaders.vi"("client handle"=w827, "error in (no error)"=w820) -> ("client handle out"=w826:T6, "headers"=w825:string, "error out"=w818:errorcluster)  [unwired: 11 in]
          n304 = Compound Arithmetic op=AND ("Mehrfacharithmetik")(invert w818, w817, w816) -> (w815:bool)
        }
        frame "Seriennummer: Update step states" {
          w871 = string[] ["\"\"", "\"00AB1234\""]
          w872 = string[] ["\"ok\"", "\"fail\""]
          # "/r/seriennummer/{seriennummer}/update_step"
          n305 = call "LabVIEW.FGV.Store_ID.vi"("Command"=enum16{"clear", "write", "read"}."read", "error in (no error)"=w895) -> ("Step IDs out[]"=w881:string[], "Step types out[]"=w880:string[], "error out"=w894:errorcluster)  [unwired: 8 in, 3 out]
          n306 = Concatenate Strings(w891, "/r/seriennummer/" ("String"), w889, "/update_step" ("String")) -> (w861:string)
          n307 = for {
            N: 2 -> [_]
            tunnel: w861 -> [w918]
            shift-right: [w917] -> w887
            shift-left: w893 -> [w919]
            shift-right: [w912] -> w877
            shift-left: w894 -> [w920]
            tunnel: w881 -> [w910] mode=indexing
            tunnel: w880 -> [w911] mode=indexing
            tunnel: w872 -> [w909] mode=indexing
            tunnel: w871 -> [w908] mode=indexing
            tunnel: [w906] -> w879 mode=indexing
            tunnel: [w905] -> w863
            tunnel: [w904] -> w862
            tunnel: [w903] -> w860
            n308 = Build Array(w911, w910, w909, w908) -> (w907:string[])
            n309 = call "LabVIEW.Service.JSON_Input.vi"("Command"=LabVIEW.Service.JSON_Input_Command."Serial number update step", "Fehler (Eingang, kein Fehler)"=w920, "Value[]"=w907) -> ("Fehler (Ausgang)"=w915:errorcluster, "<JSON>"=w903:string)  [unwired: 7 in]
            n310 = call-poly <vilib>:"POST.vi"("client handle"=w919, "url"=w918, "buffer"=w903, "error in (no error)"=w915) -> ("client handle out"=w917:T6, "headers"=w904:string, "body"=w905:string, "error out"=w912:errorcluster)  [unwired: 8 in]
            n311 = Match Pattern(string=w904, regular expression="200 OK" ("Regulärer Ausdruck")) -> (offset past match=w913:i32)  [unwired: 1 in, 3 out]
            n312 = Greater Than 0?(x=w913) -> (x > 0?=w906:bool)
          }
          n313 = And Array Elements(Boolean array=w879) -> (logical AND=w864:bool)
          n314 = call <vilib>:"Find Multiple Items.vi"("$Path or Item Name"="$.steps[*].state", "error in (no error)"=w877, "JSON"=w863) -> ("error out"=w875:errorcluster, "<JSON>"=w874:string[])  [unwired: 5 in, 2 out]
          n315 = call <vilib>:"Find Multiple Items.vi"("$Path or Item Name"="$.steps[*].value", "error in (no error)"=w875, "JSON"=w863) -> ("error out"=w869:errorcluster, "<JSON>"=w873:string[])  [unwired: 5 in, 2 out]
          n316 = for {
            N: 2 -> [_]
            tunnel: w874 -> [w902] mode=indexing
            tunnel: w873 -> [w900] mode=indexing
            tunnel: w872 -> [w901] mode=indexing
            tunnel: w871 -> [w899] mode=indexing
            tunnel: [w898] -> w868 mode=indexing
            tunnel: [w897] -> w866 mode=indexing
            n317 = Equal?(x=w900, y=w899) -> (x = y?=w897:bool)
            n318 = Equal?(x=w902, y=w901) -> (x = y?=w898:bool)
          }
          n319 = call <vilib>:"ListHeaders.vi"("client handle"=w887, "error in (no error)"=w869) -> ("client handle out"=w886:T6, "headers"=w885:string, "error out"=w884:errorcluster)  [unwired: 11 in]
          n320 = And Array Elements(Boolean array=w868) -> (logical AND=w867:bool)
          n321 = And Array Elements(Boolean array=w866) -> (logical AND=w865:bool)
          n322 = Compound Arithmetic op=AND ("Mehrfacharithmetik")(invert w884, w867, w865, w864) -> (w883:bool)
        }
        frame "Seriennummer: Get data and steps" {
          w942 = "\"" ("String")
          # "/r/seriennummer/{seriennummer}"
          n323 = Concatenate Strings(w962, "/r/seriennummer/", w943) -> (w931:string)
          n324 = Concatenate Strings(w942, w943, w942) -> (w941:string)
          n325 = call <vilib>:"GET.vi"("client handle"=w967, "url"=w931, "error in (no error)"=w963) -> ("client handle out"=w966:T6, "headers"=w956:string, "body"=w926:string, "error out"=w960:errorcluster)  [unwired: 9 in]
          n326 = call <vilib>:"Find Item.vi"("$Path or Item Name"="infoText", "error in (no error)"=w960, "JSON"=w926) -> ("error out"=w939:errorcluster, "<JSON>"=w955:string)  [unwired: 5 in, 2 out]
          n327 = call <vilib>:"Find Item.vi"("$Path or Item Name"="seriennummer", "error in (no error)"=w939, "JSON"=w926) -> ("error out"=w938:errorcluster, "<JSON>"=w940:string)  [unwired: 5 in, 2 out]
          n328 = call <vilib>:"Find Multiple Items.vi"("$Path or Item Name"="$.steps[*].state", "error in (no error)"=w938, "JSON"=w926) -> ("error out"=w954:errorcluster, "<JSON>"=w948:string[])  [unwired: 5 in, 2 out]
          n329 = call <vilib>:"Find Multiple Items.vi"("$Path or Item Name"="$.steps[*].value", "error in (no error)"=w954, "JSON"=w926) -> ("error out"=w929:errorcluster, "<JSON>"=w947:string[])  [unwired: 5 in, 2 out]
          n330 = for {
            N: 2 -> [_]
            tunnel: [w977] -> w950 mode=indexing
            tunnel: [w976] -> w951 mode=indexing
            tunnel: w948 -> [w975] mode=indexing
            tunnel: w947 -> [w973] mode=indexing
            tunnel: string[] ["\"ok\"", "\"fail\""] -> [w974] mode=indexing
            tunnel: string[] ["\"\"", "\"00AB1234\""] -> [w972] mode=indexing
            n331 = Equal?(x=w975, y=w974) -> (x = y?=w977:bool)
            n332 = Equal?(x=w973, y=w972) -> (x = y?=w976:bool)
          }
          n333 = call <vilib>:"Find Multiple Items.vi"("$Path or Item Name"="$.steps[*].id", "error in (no error)"=w929, "JSON"=w926) -> ("error out"=w927:errorcluster, "<JSON>"=w923:string[])  [unwired: 5 in, 2 out]
          n334 = call <vilib>:"Find Multiple Items.vi"("$Path or Item Name"="$.steps[*].type", "error in (no error)"=w927, "JSON"=w926) -> ("error out"=w924:errorcluster, "<JSON>"=w922:string[])  [unwired: 5 in, 2 out]
          n335 = And Array Elements(Boolean array=w950) -> (logical AND=w936:bool)
          n336 = And Array Elements(Boolean array=w951) -> (logical AND=w935:bool)
          n337 = Match Pattern(string=w956, regular expression="200 OK" ("Regulärer Ausdruck")) -> (offset past match=w970:i32)  [unwired: 1 in, 3 out]
          n338 = call "LabVIEW.FGV.Store_ID.vi"("Command"=enum16{"clear", "write", "read"}."write", "Step IDs in[]"=w923, "Step types in[]"=w922, "error in (no error)"=w924) -> ("error out"=w921:errorcluster)  [unwired: 6 in, 5 out]
          n339 = Greater Than 0?(x=w970) -> (x > 0?=w969:bool)
          n340 = Equal?(x=w940, y=w941) -> (x = y?=w933:bool)
          n341 = Equal?(x=w955, y=w937) -> (x = y?=w932:bool)
          n342 = call <vilib>:"ListHeaders.vi"("client handle"=w966, "error in (no error)"=w921) -> ("client handle out"=w965:T6, "headers"=w959:string, "error out"=w957:errorcluster)  [unwired: 11 in]
          n343 = And(x=w936, y=w935) -> (x .and. y?=w934:bool)
          n344 = Compound Arithmetic op=AND ("Mehrfacharithmetik")(invert w957, w969, w933) -> (w958:bool)
        }
        frame "Seriennummer: Get all label configurations" {
          # "/r/seriennummer/{seriennummer}/labels"
          n345 = Concatenate Strings(w1003, "/r/seriennummer/", w990, "/labels" ("String")) -> (w978:string)
          n346 = call <vilib>:"GET.vi"("client handle"=w1004, "url"=w978, "error in (no error)"=w1005) -> ("client handle out"=w999:T6, "headers"=w994:string, "body"=w986:string, "error out"=w987:errorcluster)  [unwired: 9 in]
          n347 = call <vilib>:"Get Array Elements.vi"("error in (no error)"=w987, "JSON"=w986) -> ("error out"=w984:errorcluster, "<JSON>"=w989:string[])  [unwired: 7 in, 1 out]
          n348 = Index Array(array=w989, index=0 ("Index")) -> (element=w985:string)
          n349 = call <vilib>:"Find Item.vi"("$Path or Item Name"="name", "error in (no error)"=w984, "JSON"=w985) -> ("error out"=w997:errorcluster, "<JSON>"=w983:string)  [unwired: 5 in, 2 out]
          n350 = call <vilib>:"ListHeaders.vi"("client handle"=w999, "error in (no error)"=w997) -> ("client handle out"=w998:T6, "headers"=w996:string, "error out"=w993:errorcluster)  [unwired: 11 in]
          n351 = Match Pattern(string=w994, regular expression="200 OK" ("Regulärer Ausdruck")) -> (offset past match=w981:i32)  [unwired: 1 in, 3 out]
          n352 = Match Pattern(string=w983, regular expression="OHB" ("Regulärer Ausdruck")) -> (offset past match=w980:i32)  [unwired: 1 in, 3 out]
          n353 = Greater Than 0?(x=w980) -> (x > 0?=w979:bool)
          n354 = Greater Than 0?(x=w981) -> (x > 0?=w992:bool)
          n355 = Compound Arithmetic op=AND ("Mehrfacharithmetik")(invert w993, w992, w979) -> (w991:bool)
        }
        frame "Seriennummer: Create a text report(Prüfbericht)" {
          w1014 = TRUE ("Alle ersetzen? (F)")
          # "/r/seriennummer/{seriennummer}/report"
          n356 = Concatenate Strings(w1055, "/r/seriennummer/" ("String"), w1037, "/report" ("String")) -> (w1007:string)
          n357 = call-poly <vilib>:"POST.vi"("client handle"=w1053, "url"=w1007, "error in (no error)"=w1054) -> ("client handle out"=w1051:T6, "headers"=w1045:string, "body"=w1017:string, "error out"=w1042:errorcluster)  [unwired: 9 in]
          n358 = call <vilib>:"Find Multiple Items.vi"("$Path or Item Name"="$.reports[*].fileName", "error in (no error)"=w1042, "JSON"=w1017) -> ("error out"=w1010:errorcluster, "<JSON>"=w1039:string[])  [unwired: 5 in, 2 out]
          n359 = Array Size(array=w1039) -> (size(s)=w1041:i32)
          n360 = Decrement(x=w1041) -> (x-1=w1040:i32)
          n361 = Index Array(array=w1039, index=w1040) -> (element=w1011:string)
          n362 = Search and Replace String(replace all?=w1014, case sensitive?=w1014, input string=w1011, search string="\"" ("Such-String"), replace string="", error in=w1010) -> (result string=w1009:string, error out=w1008:errorcluster)  [unwired: 2 in, 2 out]
          n363 = call "LabVIEW.FGV.Store_ID.vi"("Command"=enum16{"clear", "write", "read"}."write", "error in (no error)"=w1008, "File Name In"=w1009) -> ("error out"=w1015:errorcluster)  [unwired: 7 in, 5 out]
          n364 = Match Pattern(string=w1009, regular expression=w1038) -> (offset past match=w1029:i32)  [unwired: 1 in, 3 out]
          n365 = Match Pattern(string=w1009, regular expression=w1037) -> (offset past match=w1028:i32)  [unwired: 1 in, 3 out]
          n366 = Match Pattern(string=w1009, regular expression=w1036) -> (offset past match=w1027:i32)  [unwired: 1 in, 3 out]
          n367 = Match Pattern(string=w1009, regular expression="FEHLER" ("Regulärer Ausdruck")) -> (offset past match=w1026:i32)  [unwired: 1 in, 3 out]
          n368 = Greater Than 0?(x=w1029) -> (x > 0?=w1023:bool)
          n369 = Greater Than 0?(x=w1028) -> (x > 0?=w1022:bool)
          n370 = Greater Than 0?(x=w1027) -> (x > 0?=w1021:bool)
          n371 = Greater Than 0?(x=w1026) -> (x > 0?=w1020:bool)
          n372 = call <vilib>:"Find Multiple Items.vi"("$Path or Item Name"="$.reports[*].result", "error in (no error)"=w1015, "JSON"=w1017) -> ("error out"=w1030:errorcluster, "<JSON>"=w1031:string[])  [unwired: 5 in, 2 out]
          n373 = Array Size(array=w1031) -> (size(s)=w1032:i32)
          n374 = Decrement(x=w1032) -> (x-1=w1033:i32)
          n375 = Index Array(array=w1031, index=w1033) -> (element=w1025:string)
          n376 = Equal?(x=w1025, y="\"in_progress_with_failed_step\"" ("Regulärer Ausdruck")) -> (x = y?=w1019:bool)
          n377 = Match Pattern(string=w1045, regular expression="200 OK" ("Regulärer Ausdruck")) -> (offset past match=w1048:i32)  [unwired: 1 in, 3 out]
          n378 = call <vilib>:"ListHeaders.vi"("client handle"=w1051, "error in (no error)"=w1030) -> ("client handle out"=w1052:T6, "headers"=w1050:string, "error out"=w1046:errorcluster)  [unwired: 11 in]
          n379 = Greater Than 0?(x=w1048) -> (x > 0?=w1044:bool)
          n380 = Compound Arithmetic op=AND ("Mehrfacharithmetik")(invert w1046, w1044, w1023, w1022, w1021, w1020, w1019) -> (w1018:bool)
        }
        frame "Seriennummer: Get the text report(Prüfbericht)" {
          # "/r/seriennummer/{seriennummer}/report/{fileName}"
          n381 = call "LabVIEW.FGV.Store_ID.vi"("Command"=enum16{"clear", "write", "read"}."read", "error in (no error)"=w1085) -> ("File Name Out"=w1081:string, "error out"=w1082:errorcluster)  [unwired: 8 in, 4 out]
          n382 = Concatenate Strings(w1087, "/r/seriennummer/", w1086, "/report/", w1081) -> (w1067:string)
          n383 = call <vilib>:"GET.vi"("client handle"=w1088, "url"=w1067, "error in (no error)"=w1082) -> ("client handle out"=w1079:T6, "headers"=w1073:string, "body"=w1066:string, "error out"=w1080:errorcluster)  [unwired: 9 in]
          n384 = Match Pattern(string=w1066, regular expression="03." ("Regulärer Ausdruck")) -> (after substring=w1063:string)  [unwired: 1 in, 3 out]
          n385 = Match Pattern(string=w1063, regular expression="04." ("Regulärer Ausdruck")) -> (before substring=w1061:string)  [unwired: 1 in, 3 out]
          n386 = Match Pattern(string=w1066, regular expression="00AB1234" ("Regulärer Ausdruck")) -> (offset past match=w1068:i32)  [unwired: 1 in, 3 out]
          n387 = Match Pattern(string=w1073, regular expression="200 OK" ("Regulärer Ausdruck")) -> (offset past match=w1075:i32)  [unwired: 1 in, 3 out]
          n388 = Match Pattern(string=w1061, regular expression="OK" ("Regulärer Ausdruck")) -> (offset past match=w1060:i32)  [unwired: 1 in, 3 out]
          n389 = call <vilib>:"ListHeaders.vi"("client handle"=w1079, "error in (no error)"=w1080) -> ("client handle out"=w1078:T6, "headers"=w1076:string, "error out"=w1072:errorcluster)  [unwired: 11 in]
          n390 = Greater Than 0?(x=w1075) -> (x > 0?=w1071:bool)
          n391 = Greater Than 0?(x=w1068) -> (x > 0?=w1058:bool)
          n392 = Greater Than 0?(x=w1060) -> (x > 0?=w1059:bool)
          n393 = Compound Arithmetic op=AND ("Mehrfacharithmetik")(invert w1072, w1071, w1058) -> (w1070:bool)
        }
        frame "Seriennummer: Delete the text report(Prüfbericht)" {
          # "/r/seriennummer/{seriennummer}/report/{fileName}"
          n394 = call "LabVIEW.FGV.Store_ID.vi"("Command"=enum16{"clear", "write", "read"}."read", "error in (no error)"=w1101) -> ("File Name Out"=w1096:string, "error out"=w1110:errorcluster)  [unwired: 8 in, 4 out]
          n395 = Concatenate Strings(w1098, "/r/seriennummer/", w1097, "/report/", w1096) -> (w1090:string)
          n396 = call <vilib>:"DELETE.vi"("client handle"=w1104, "url"=w1090, "error in (no error)"=w1110) -> ("client handle out"=w1103:T6, "headers"=w1095:string, "body"=w1094:string, "error out"=w1106:errorcluster)  [unwired: 9 in]
          n397 = call "LabVIEW.FGV.Store_ID.vi"("Command"=enum16{"clear", "write", "read"}."clear", "error in (no error)"=w1106) -> ("error out"=w1105:errorcluster)  [unwired: 8 in, 5 out]
          n398 = Match Pattern(string=w1095, regular expression="204" ("Regulärer Ausdruck")) -> (offset past match=w1108:i32)  [unwired: 1 in, 3 out]
          n399 = call <vilib>:"ListHeaders.vi"("client handle"=w1103, "error in (no error)"=w1105) -> ("client handle out"=w1102:T6, "headers"=w1092:string, "error out"=w1093:errorcluster)  [unwired: 11 in]
          n400 = Greater Than 0?(x=w1108) -> (x > 0?=w1091:bool)
        }
        frame "Seriennummer: Upload a document(txt file)" {
          w1144 = "\"" ("String")
          w1114 = "Test_Document.txt" ("String")
          n401 = control-ref of="Dieses VI"() -> (w1117:refnum<vi>)
          n402 = call "LabVIEW.Service.File_path.vi"("Fehler (Eingang, kein Fehler)"=w1116, "File name"=w1114, "VI Reference"=w1117) -> ("Fehler (Ausgang)"=w1115:errorcluster, "Dateipfad-Bedienelement"=w1113:path)  [unwired: 7 in]
          n403 = Concatenate Strings(w1164, "/r/seriennummer/", w1162, "/file" ("String")) -> (w1119:string)
          n404 = Strip Path(path=w1113) -> (name=w1159:string)  [unwired: 1 out]
          n405 = call <vilib>:"AddHeader.vi"("client handle"=w1165, "header"="Content-Type", "value"="multipart/form-data", "error in (no error)"=w1115) -> ("client handle out"=w1153:T6, "error out"=w1152:errorcluster)  [unwired: 10 in]
          n406 = Bundle By Name(cluster=T4 {"Name"="serial", "Value"="04IA01267", "File"=path "", "Filename"="", "MIME type"="application/octet-stream"} ("Element"), "Name"="file", "Value"="", "File"=w1113, "Filename"=w1159, "MIME type"="text/plain") -> (w1155:T4)
          n407 = Build Array(w1155) -> (w1118:T7)
          n408 = call <vilib>:"POSTMultipart.vi"("client handle"=w1153, "url"=w1119, "data"=w1118, "error in (no error)"=w1152) -> ("client handle out"=w1135:T6, "headers"=w1147:string, "body"=w1124:string, "error out"=w1145:errorcluster)  [unwired: 8 in]
          n409 = call <vilib>:"Find Multiple Items.vi"("$Path or Item Name"="$.documents[*].fileName", "error in (no error)"=w1145, "JSON"=w1124) -> ("error out"=w1132:errorcluster, "<JSON>"=w1121:string[])  [unwired: 5 in, 2 out]
          n410 = call <vilib>:"Find Multiple Items.vi"("$Path or Item Name"="$.documents[*].id", "error in (no error)"=w1132, "JSON"=w1124) -> ("error out"=w1126:errorcluster, "<JSON>"=w1128:string[])  [unwired: 5 in, 2 out]
          n411 = Array Size(array=w1128) -> (size(s)=w1130:i32)
          n412 = Array Size(array=w1121) -> (size(s)=w1123:i32)
          n413 = Decrement(x=w1130) -> (x-1=w1129:i32)
          n414 = Decrement(x=w1123) -> (x-1=w1122:i32)
          n415 = Index Array(array=w1128, index=w1129) -> (element=w1127:string)
          n416 = call "LabVIEW.FGV.Store_ID.vi"("ID In"=w1127, "Command"=enum16{"clear", "write", "read"}."write", "error in (no error)"=w1126) -> ("error out"=w1125:errorcluster)  [unwired: 7 in, 5 out]
          n417 = Index Array(array=w1121, index=w1122) -> (element=w1120:string)
          n418 = Concatenate Strings(w1144, w1114, w1144) -> (w1143:string)
          n419 = Match Pattern(string=w1147, regular expression="201" ("Regulärer Ausdruck")) -> (offset past match=w1148:i32)  [unwired: 1 in, 3 out]
          n420 = call <vilib>:"AddHeader.vi"("client handle"=w1135, "header"="Content-Type", "value"="application/json", "error in (no error)"=w1125) -> ("client handle out"=w1134:T6, "error out"=w1136:errorcluster)  [unwired: 10 in]
          n421 = Equal?(x=w1120, y=w1143) -> (x = y?=w1140:bool)
          n422 = Greater Than 0?(x=w1148) -> (x > 0?=w1141:bool)
          n423 = call <vilib>:"ListHeaders.vi"("client handle"=w1134, "error in (no error)"=w1136) -> ("client handle out"=w1151:T6, "headers"=w1150:string, "error out"=w1142:errorcluster)  [unwired: 11 in]
          n424 = Compound Arithmetic op=AND ("Mehrfacharithmetik")(invert w1142, w1141, w1140) -> (w1139:bool)
        }
        frame "Seriennummer: Get the document" {
          # "/r/seriennummer/{seriennummer}/file/{documentID}"
          n425 = call "LabVIEW.FGV.Store_ID.vi"("Command"=enum16{"clear", "write", "read"}."read", "error in (no error)"=w1190) -> ("ID Out"=w1183:string, "error out"=w1189:errorcluster)  [unwired: 8 in, 4 out]
          n426 = Concatenate Strings(w1185, "/r/seriennummer/", w1184, "/file/", w1183) -> (w1168:string)
          n427 = call <vilib>:"GET.vi"("client handle"=w1188, "url"=w1168, "error in (no error)"=w1189) -> ("client handle out"=w1181:T6, "headers"=w1176:string, "body"=w1172:string, "error out"=w1182:errorcluster)  [unwired: 9 in]
          n428 = call <vilib>:"ListHeaders.vi"("client handle"=w1181, "error in (no error)"=w1182) -> ("client handle out"=w1180:T6, "headers"=w1169:string, "error out"=w1175:errorcluster)  [unwired: 11 in]
          n429 = Match Pattern(string=w1176, regular expression="200 OK" ("Regulärer Ausdruck")) -> (offset past match=w1177:i32)  [unwired: 1 in, 3 out]
          n430 = Greater Than 0?(x=w1177) -> (x > 0?=w1173:bool)
          n431 = Equal?(x=w1172, y="Test") -> (x = y?=w1170:bool)
          n432 = Compound Arithmetic op=AND ("Mehrfacharithmetik")(invert w1175, w1173, w1170) -> (w1174:bool)
        }
        frame "Seriennummer: Get the document thumbnail" {
          # "/r/seriennummer/{seriennummer}/file/{documentID}/thumbnail"
          n433 = call "LabVIEW.FGV.Store_ID.vi"("Command"=enum16{"clear", "write", "read"}."read", "error in (no error)"=w1217) -> ("ID Out"=w1210:string, "error out"=w1216:errorcluster)  [unwired: 8 in, 4 out]
          n434 = Concatenate Strings(w1212, "/r/seriennummer/", w1211, "/file/", w1210, "/thumbnail" ("String")) -> (w1192:string)
          n435 = call <vilib>:"GET.vi"("client handle"=w1215, "url"=w1192, "error in (no error)"=w1216) -> ("client handle out"=w1208:T6, "headers"=w1203:string, "body"=w1197:string, "error out"=w1209:errorcluster)  [unwired: 9 in]
          n436 = call <vilib>:"ListHeaders.vi"("client handle"=w1208, "error in (no error)"=w1209) -> ("client handle out"=w1207:T6, "headers"=w1199:string, "error out"=w1202:errorcluster)  [unwired: 11 in]
          n437 = Match Pattern(string=w1197, regular expression="ÿØ" ("Regulärer Ausdruck")) -> (offset past match=w1195:i32)  [unwired: 1 in, 3 out]
          n438 = Match Pattern(string=w1203, regular expression="200 OK" ("Regulärer Ausdruck")) -> (offset past match=w1204:i32)  [unwired: 1 in, 3 out]
          n439 = Greater Than 0?(x=w1204) -> (x > 0?=w1200:bool)
          n440 = Equal?(x=w1195, y=2) -> (x = y?=w1193:bool)
          n441 = Compound Arithmetic op=AND ("Mehrfacharithmetik")(invert w1202, w1200, w1193) -> (w1201:bool)
        }
        frame "Seriennummer: Delete the document" {
          # "/r/seriennummer/{seriennummer}/file/{documentID}"
          n442 = call "LabVIEW.FGV.Store_ID.vi"("Command"=enum16{"clear", "write", "read"}."read", "error in (no error)"=w1236) -> ("ID Out"=w1226:string, "error out"=w1247:errorcluster)  [unwired: 8 in, 4 out]
          n443 = Concatenate Strings(w1235, "/r/seriennummer/", w1232, "/file/", w1226) -> (w1219:string)
          n444 = call <vilib>:"DELETE.vi"("client handle"=w1239, "url"=w1219, "error in (no error)"=w1247) -> ("client handle out"=w1238:T6, "headers"=w1233:string, "body"=w1228:string, "error out"=w1230:errorcluster)  [unwired: 9 in]
          n445 = call <vilib>:"Find Multiple Items.vi"("$Path or Item Name"="$.documents[*].id", "error in (no error)"=w1230, "JSON"=w1228) -> ("error out"=w1229:errorcluster, "<JSON>"=w1227:string[])  [unwired: 5 in, 2 out]
          n446 = call "LabVIEW.FGV.Store_ID.vi"("Command"=enum16{"clear", "write", "read"}."clear", "error in (no error)"=w1229) -> ("error out"=w1243:errorcluster)  [unwired: 8 in, 5 out]
          n447 = Search 1D Array(1D array=w1227, element=w1226) -> (index of element=w1225:i32)  [unwired: 1 in]
          n448 = Match Pattern(string=w1233, regular expression="200 OK" ("Regulärer Ausdruck")) -> (offset past match=w1245:i32)  [unwired: 1 in, 3 out]
          n449 = call <vilib>:"ListHeaders.vi"("client handle"=w1238, "error in (no error)"=w1243) -> ("client handle out"=w1237:T6, "headers"=w1234:string, "error out"=w1222:errorcluster)  [unwired: 11 in]
          n450 = Greater Than 0?(x=w1245) -> (x > 0?=w1221:bool)
          n451 = Equal?(x=w1225, y=-1) -> (x = y?=w1223:bool)
          n452 = Compound Arithmetic op=AND ("Mehrfacharithmetik")(invert w1222, w1221, w1223) -> (w1220:bool)
        }
        frame "Seriennummer: Bulk lookup" {
          w1266 = "\"" ("String")
          w1268 = "\"" ("String")
          w1281 = "\"" ("String")
          w1283 = "\"" ("String")
          # "/r/seriennummer/bulk_lookup"
          n453 = Concatenate Strings(w1266, w1265, w1266) -> (w1263:string)
          n454 = Concatenate Strings(w1281, w1280, w1281) -> (w1278:string)
          n455 = Concatenate Strings(w1283, w1282, w1283) -> (w1279:string)
          n456 = Concatenate Strings(w1268, w1267, w1268) -> (w1264:string)
          n457 = Build Array(w1279, w1278) -> (w1254:string[])
          n458 = Build Array(w1264, w1263) -> (w1261:string[])
          n459 = call "LabVIEW.Service.JSON_Input.vi"("Command"=LabVIEW.Service.JSON_Input_Command."Serial number bulk lookup", "Fehler (Eingang, kein Fehler)"=w1286, "Value[]"=w1254) -> ("Fehler (Ausgang)"=w1285:errorcluster, "<JSON>"=w1249:string)  [unwired: 7 in]
          n460 = Concatenate Strings(w1289, "/r/seriennummer/" ("String"), "bulk_lookup" ("String")) -> (w1250:string)
          n461 = call-poly <vilib>:"POST.vi"("client handle"=w1293, "url"=w1250, "buffer"=w1249, "error in (no error)"=w1285) -> ("client handle out"=w1292:T6, "headers"=w1272:string, "body"=w1253:string, "error out"=w1276:errorcluster)  [unwired: 8 in]
          n462 = call <vilib>:"Find Multiple Items.vi"("$Path or Item Name"="$.results[*].seriennummer", "error in (no error)"=w1276, "JSON"=w1253) -> ("error out"=w1252:errorcluster, "<JSON>"=w1269:string[])  [unwired: 5 in, 2 out]
          n463 = Equal?(x=w1269, y=w1254) -> (x = y?=w1258:bool[])
          n464 = call <vilib>:"Find Multiple Items.vi"("$Path or Item Name"="$.results[*].produkt", "error in (no error)"=w1252, "JSON"=w1253) -> ("error out"=w1270:errorcluster, "<JSON>"=w1262:string[])  [unwired: 5 in, 2 out]
          n465 = Equal?(x=w1262, y=w1261) -> (x = y?=w1257:bool[])
          n466 = And Array Elements(Boolean array=w1258) -> (logical AND=w1256:bool)
          n467 = And Array Elements(Boolean array=w1257) -> (logical AND=w1251:bool)
          n468 = call <vilib>:"ListHeaders.vi"("client handle"=w1292, "error in (no error)"=w1270) -> ("client handle out"=w1291:T6, "headers"=w1275:string, "error out"=w1260:errorcluster)  [unwired: 11 in]
          n469 = Match Pattern(string=w1272, regular expression="200 OK" ("Regulärer Ausdruck")) -> (offset past match=w1273:i32)  [unwired: 1 in, 3 out]
          n470 = Greater Than 0?(x=w1273) -> (x > 0?=w1259:bool)
          n471 = Compound Arithmetic op=AND ("Mehrfacharithmetik")(invert w1260, w1259, w1256, w1251) -> (w1255:bool)
        }
        frame "Vorgang: Update the description text" {
          # "/r/vorgang/{vNr}/infotext"
          n472 = Concatenate Strings(w1312, "/r/vorgang/", w1308, "/infotext" ("String")) -> (w1295:string)
          n473 = call "LabVIEW.Service.JSON_Input.vi"("Command"=LabVIEW.Service.JSON_Input_Command."Serial number info text", "Fehler (Eingang, kein Fehler)"=w1313, "Value 1"=w1309) -> ("Fehler (Ausgang)"=w1315:errorcluster, "<JSON>"=w1294:string)  [unwired: 7 in]
          n474 = call-poly <vilib>:"PUT.vi"("client handle"=w1311, "url"=w1295, "buffer"=w1294, "error in (no error)"=w1315) -> ("client handle out"=w1306:T6, "headers"=w1301:string, "body"=w1303:string, "error out"=w1299:errorcluster)  [unwired: 8 in]
          n475 = Match Pattern(string=w1301, regular expression="204" ("Regulärer Ausdruck")) -> (offset past match=w1300:i32)  [unwired: 1 in, 3 out]
          n476 = Greater Than 0?(x=w1300) -> (x > 0?=w1297:bool)
          n477 = call <vilib>:"ListHeaders.vi"("client handle"=w1306, "error in (no error)"=w1299) -> ("client handle out"=w1305:T6, "headers"=w1304:string, "error out"=w1298:errorcluster)  [unwired: 11 in]
          n478 = Compound Arithmetic op=AND ("Mehrfacharithmetik")(invert w1298, w1297) -> (w1296:bool)
        }
        frame "Vorgang: Migrate serial numbers to a Vorgang" {
          w1326 = "\"" ("String")
          w1333 = "\"" ("String")
          # "/r/vorgang/migrate"
          n479 = Concatenate Strings(w1326, w1319, w1326) -> (w1325:string)
          n480 = Concatenate Strings(w1333, w1332, w1333) -> (w1323:string)
          n481 = Build Array(w1325) -> (w1324:string[])
          n482 = call "LabVIEW.Service.JSON_Input.vi"("Command"=LabVIEW.Service.JSON_Input_Command."Vorgang migrate serial numbers to Vorgang", "Fehler (Eingang, kein Fehler)"=w1334, "Value[]"=w1324, "Value 1"=w1323) -> ("Fehler (Ausgang)"=w1343:errorcluster, "<JSON>"=w1317:string)  [unwired: 6 in]
          n483 = Concatenate Strings(w1335, "/r/vorgang/migrate" ("String")) -> (w1318:string)
          n484 = call-poly <vilib>:"POST.vi"("client handle"=w1342, "url"=w1318, "buffer"=w1317, "error in (no error)"=w1343) -> ("client handle out"=w1339:T6, "headers"=w1328:string, "body"=w1331:string, "error out"=w1327:errorcluster)  [unwired: 8 in]
          n485 = Match Pattern(string=w1328, regular expression="204" ("Regulärer Ausdruck")) -> (offset past match=w1329:i32)  [unwired: 1 in, 3 out]
          n486 = call <vilib>:"ListHeaders.vi"("client handle"=w1339, "error in (no error)"=w1327) -> ("client handle out"=w1338:T6, "headers"=w1337:string, "error out"=w1321:errorcluster)  [unwired: 11 in]
          n487 = Greater Than 0?(x=w1329) -> (x > 0?=w1322:bool)
          n488 = Compound Arithmetic op=AND ("Mehrfacharithmetik")(invert w1321, w1322) -> (w1320:bool)
        }
        frame "Vorgang: Migrate serial numbers to a product revision" {
          w1360 = "\"" ("String")
          w1362 = "\"" ("String")
          w1365 = "\"" ("String")
          # "/r/vorgang/{vNr}/change_revision"
          n489 = Concatenate Strings(w1360, w1359, w1360) -> (w1358:string)
          n490 = Concatenate Strings(w1362, w1346, w1362) -> (w1361:string)
          n491 = Concatenate Strings(w1365, w1364, w1365) -> (w1363:string)
          n492 = Build Array(w1358) -> (w1357:string[])
          n493 = call "LabVIEW.Service.JSON_Input.vi"("Command"=LabVIEW.Service.JSON_Input_Command."Vorgang migrate serial numbers to product revision", "Fehler (Eingang, kein Fehler)"=w1370, "Value[]"=w1357, "Value 1"=w1363, "Value 2"=w1361) -> ("Fehler (Ausgang)"=w1375:errorcluster, "<JSON>"=w1344:string)  [unwired: 5 in]
          n494 = Concatenate Strings(w1371, "/r/vorgang/" ("String"), w1348, "/change_revision" ("String")) -> (w1345:string)
          n495 = call-poly <vilib>:"POST.vi"("client handle"=w1369, "url"=w1345, "buffer"=w1344, "error in (no error)"=w1375) -> ("client handle out"=w1368:T6, "headers"=w1353:string, "body"=w1354:string, "error out"=w1349:errorcluster)  [unwired: 8 in]
          n496 = Match Pattern(string=w1353, regular expression="204" ("Regulärer Ausdruck")) -> (offset past match=w1355:i32)  [unwired: 1 in, 3 out]
          n497 = call <vilib>:"ListHeaders.vi"("client handle"=w1368, "error in (no error)"=w1349) -> ("client handle out"=w1367:T6, "headers"=w1366:string, "error out"=w1351:errorcluster)  [unwired: 11 in]
          n498 = Greater Than 0?(x=w1355) -> (x > 0?=w1352:bool)
          n499 = Compound Arithmetic op=AND ("Mehrfacharithmetik")(invert w1351, w1352) -> (w1350:bool)
        }
        frame "Vorgang: Update step states" {
          # "/r/vorgang/{vNr}/{produkt}/bulk_edit_steps"
          n500 = call "LabVIEW.FGV.Store_ID.vi"("Command"=enum16{"clear", "write", "read"}."read", "error in (no error)"=w1396) -> ("Step IDs out[]"=w1395:string[], "Step types out[]"=w1392:string[], "error out"=w1385:errorcluster)  [unwired: 8 in, 3 out]
          n501 = Index Array(array=w1395, index=2 ("Index")) -> (element=w1390:string)
          n502 = Index Array(array=w1392, index=2 ("Index")) -> (element=w1391:string)
          n503 = Build Array(w1391, w1390, "true" ("Element"), "null" ("Element")) -> (w1387:string[])
          n504 = call "LabVIEW.Service.JSON_Input.vi"("Command"=LabVIEW.Service.JSON_Input_Command."Vorgang Update step states", "Fehler (Eingang, kein Fehler)"=w1385, "Value[]"=w1387) -> ("Fehler (Ausgang)"=w1410:errorcluster, "<JSON>"=w1376:string)  [unwired: 7 in]
          n505 = Concatenate Strings(w1402, "/r/vorgang/" ("String"), w1401, "/" ("String"), w1399, "/bulk_edit_steps" ("String")) -> (w1377:string)
          n506 = call-poly <vilib>:"POST.vi"("client handle"=w1407, "url"=w1377, "buffer"=w1376, "error in (no error)"=w1410) -> ("client handle out"=w1405:T6, "headers"=w1378:string, "body"=w1384:string, "error out"=w1386:errorcluster)  [unwired: 8 in]
          n507 = call <vilib>:"ListHeaders.vi"("client handle"=w1405, "error in (no error)"=w1386) -> ("client handle out"=w1404:T6, "headers"=w1403:string, "error out"=w1380:errorcluster)  [unwired: 11 in]
          n508 = Match Pattern(string=w1378, regular expression="204" ("Regulärer Ausdruck")) -> (offset past match=w1382:i32)  [unwired: 1 in, 3 out]
          n509 = Greater Than 0?(x=w1382) -> (x > 0?=w1381:bool)
          n510 = Compound Arithmetic op=AND ("Mehrfacharithmetik")(invert w1380, w1381) -> (w1379:bool)
        }
        frame "Vorgang: Create test reports(Prüfprotokoll)" {
          # "/r/vorgang/{vNr}/{produkt}/bulk_create_reports"
          n511 = Concatenate Strings(w1425, "/r/vorgang/" ("String"), w1424, "/" ("String"), w1422, "/bulk_create_reports" ("String")) -> (w1411:string)
          n512 = call-poly <vilib>:"POST.vi"("client handle"=w1430, "url"=w1411, "error in (no error)"=w1412) -> ("client handle out"=w1428:T6, "headers"=w1413:string, "body"=w1419:string, "error out"=w1420:errorcluster)  [unwired: 9 in]
          n513 = call <vilib>:"ListHeaders.vi"("client handle"=w1428, "error in (no error)"=w1420) -> ("client handle out"=w1427:T6, "headers"=w1426:string, "error out"=w1415:errorcluster)  [unwired: 11 in]
          n514 = Match Pattern(string=w1413, regular expression="204" ("Regulärer Ausdruck")) -> (offset past match=w1417:i32)  [unwired: 1 in, 3 out]
          n515 = Greater Than 0?(x=w1417) -> (x > 0?=w1416:bool)
          n516 = Compound Arithmetic op=AND ("Mehrfacharithmetik")(invert w1415, w1416) -> (w1414:bool)
        }
        frame "Vorgang: Get basic data" {
          w1437 = "\"" ("String")
          w1450 = "\"" ("String")
          # "/r/vorgang/{vNr}"
          n517 = Concatenate Strings(w1450, w1444, w1450) -> (w1447:string)
          n518 = Concatenate Strings(w1462, "/r/vorgang/" ("String"), w1436) -> (w1432:string)
          n519 = Concatenate Strings(w1437, w1436, w1437) -> (w1434:string)
          n520 = call <vilib>:"GET.vi"("client handle"=w1465, "url"=w1432, "error in (no error)"=w1468) -> ("client handle out"=w1464:T6, "headers"=w1457:string, "body"=w1440:string, "error out"=w1456:errorcluster)  [unwired: 9 in]
          n521 = call <vilib>:"Find Item.vi"("$Path or Item Name"="vorgangInfoText", "error in (no error)"=w1456, "JSON"=w1440) -> ("error out"=w1451:errorcluster, "<JSON>"=w1454:string)  [unwired: 5 in, 2 out]
          n522 = call <vilib>:"Find Multiple Items.vi"("$Path or Item Name"="$.products[*].name", "error in (no error)"=w1451, "JSON"=w1440) -> ("error out"=w1442:errorcluster, "<JSON>"=w1449:string[])  [unwired: 5 in, 2 out]
          n523 = call <vilib>:"Find Item.vi"("$Path or Item Name"="vNr", "error in (no error)"=w1442, "JSON"=w1440) -> ("error out"=w1441:errorcluster, "<JSON>"=w1435:string)  [unwired: 5 in, 2 out]
          n524 = call <vilib>:"ListHeaders.vi"("client handle"=w1464, "error in (no error)"=w1441) -> ("client handle out"=w1467:T6, "headers"=w1466:string, "error out"=w1458:errorcluster)  [unwired: 11 in]
          n525 = Index Array(array=w1449, index=0 ("Index")) -> (element=w1448:string)
          n526 = Match Pattern(string=w1457, regular expression="200 OK" ("Regulärer Ausdruck")) -> (offset past match=w1460:i32)  [unwired: 1 in, 3 out]
          n527 = Equal?(x=w1448, y=w1447) -> (x = y?=w1438:bool)
          n528 = Equal?(x=w1435, y=w1434) -> (x = y?=w1433:bool)
          n529 = Greater Than 0?(x=w1460) -> (x > 0?=w1459:bool)
          n530 = Equal?(x=w1454, y=w1453) -> (x = y?=w1439:bool)
          n531 = Compound Arithmetic op=AND ("Mehrfacharithmetik")(invert w1458, w1459, w1433) -> (w1446:bool)
        }
        frame "Vorgang: Get serial number data and steps" {
          w1474 = TRUE ("Alle ersetzen? (F)")
          w1484 = "\"" ("String")
          # "/r/vorgang/{vNr}/{produkt}/seriennummern"
          n532 = Concatenate Strings(w1533, "/r/vorgang/" ("String"), w1532, "/" ("String"), w1531, "/seriennummern" ("String")) -> (w1475:string)
          n533 = call <vilib>:"GET.vi"("client handle"=w1538, "url"=w1475, "error in (no error)"=w1539) -> ("client handle out"=w1530:T6, "headers"=w1522:string, "body"=w1489:string, "error out"=w1491:errorcluster)  [unwired: 9 in]
          n534 = call <vilib>:"Find Multiple Items.vi"("$Path or Item Name"="$.seriennummern[*].seriennummer", "error in (no error)"=w1491, "JSON"=w1489) -> ("error out"=w1490:errorcluster, "<JSON>"=w1487:string[])  [unwired: 5 in, 2 out]
          n535 = Index Array(array=w1487, index=0 ("Index")) -> (element=w1485:string)
          n536 = Concatenate Strings(w1484, w1483, w1484) -> (w1482:string)
          n537 = call <vilib>:"Find Multiple Items.vi"("$Path or Item Name"="$.seriennummern[*].steps[*].state", "error in (no error)"=w1490, "JSON"=w1489) -> ("error out"=w1501:errorcluster, "<JSON>"=w1520:string[])  [unwired: 5 in, 2 out]
          n538 = call <vilib>:"Find Multiple Items.vi"("$Path or Item Name"="$.seriennummern[0].reports[-1].fileName", "error in (no error)"=w1501, "JSON"=w1489) -> ("error out"=w1500:errorcluster, "<JSON>"=w1480:string[])  [unwired: 5 in, 2 out]
          n539 = call <vilib>:"Find Multiple Items.vi"("$Path or Item Name"="$.seriennummern[0].fertiggemeldet", "error in (no error)"=w1500, "JSON"=w1489) -> ("error out"=w1515:errorcluster, "<JSON>"=w1511:string[])  [unwired: 5 in, 2 out]
          n540 = Index Array(array=w1511, index=0 ("Index")) -> (element=w1507:string)
          n541 = call <vilib>:"Find Multiple Items.vi"("$Path or Item Name"="$.seriennummern[0].fertigmeldungAt", "error in (no error)"=w1515, "JSON"=w1489) -> ("error out"=w1512:errorcluster, "<JSON>"=w1509:string[])  [unwired: 5 in, 2 out]
          n542 = Index Array(array=w1480, index=0 ("Index")) -> (element=w1471:string)
          n543 = Index Array(array=w1509, index=0 ("Index")) -> (element=w1506:string)
          n544 = call <vilib>:"Find Multiple Items.vi"("$Path or Item Name"="$.seriennummern[0].history[-1].fertigmeldungCSV", "error in (no error)"=w1512, "JSON"=w1489) -> ("error out"=w1499:errorcluster, "<JSON>"=w1478:string[])  [unwired: 5 in, 2 out]
          n545 = Search and Replace String(replace all?=w1474, case sensitive?=w1474, input string=w1471, search string="\"" ("Such-String"), replace string="") -> (result string=w1470:string)  [unwired: 3 in, 3 out]
          n546 = call <vilib>:"Find Multiple Items.vi"("$Path or Item Name"="$.seriennummern[*].steps[*].id", "error in (no error)"=w1499, "JSON"=w1489) -> ("error out"=w1497:errorcluster, "<JSON>"=w1494:string[])  [unwired: 5 in, 2 out]
          n547 = Index Array(array=w1478, index=0 ("Index")) -> (element=w1476:string)
          n548 = call <vilib>:"Find Multiple Items.vi"("$Path or Item Name"="$.seriennummern[*].steps[*].type", "error in (no error)"=w1497, "JSON"=w1489) -> ("error out"=w1496:errorcluster, "<JSON>"=w1493:string[])  [unwired: 5 in, 2 out]
          n549 = Build Array(w1507, w1506, w1476) -> (w1503:string[])
          n550 = Index Array(array=w1520, index=2 ("Index")) -> (element=w1518:string)
          n551 = Match Pattern(string=w1522, regular expression="200 OK" ("Regulärer Ausdruck")) -> (offset past match=w1526:i32)  [unwired: 1 in, 3 out]
          n552 = call "LabVIEW.FGV.Store_ID.vi"("Command"=enum16{"clear", "write", "read"}."write", "Step IDs in[]"=w1494, "Fertigmeldung in[]"=w1503, "Step types in[]"=w1493, "error in (no error)"=w1496, "File Name In"=w1470) -> ("error out"=w1505:errorcluster)  [unwired: 4 in, 5 out]
          n553 = Equal?(x=w1518, y="\"ok\"") -> (x = y?=w1492:bool)
          n554 = Equal?(x=w1485, y=w1482) -> (x = y?=w1481:bool)
          n555 = Greater Than 0?(x=w1526) -> (x > 0?=w1525:bool)
          n556 = call <vilib>:"ListHeaders.vi"("client handle"=w1530, "error in (no error)"=w1505) -> ("client handle out"=w1529:T6, "headers"=w1528:string, "error out"=w1523:errorcluster)  [unwired: 11 in]
          n557 = Compound Arithmetic op=AND ("Mehrfacharithmetik")(invert w1523, w1525, w1481) -> (w1524:bool)
        }
        frame "Vorgang: Get all serial numbers" {
          w1546 = "\"" ("String")
          # "/r/vorgang/{vNr}/seriennummern"
          n558 = Concatenate Strings(w1546, w1545, w1546) -> (w1543:string)
          n559 = Concatenate Strings(w1560, "/r/vorgang/" ("String"), w1559, "/seriennummern" ("String")) -> (w1540:string)
          n560 = call <vilib>:"GET.vi"("client handle"=w1562, "url"=w1540, "error in (no error)"=w1563) -> ("client handle out"=w1557:T6, "headers"=w1551:string, "body"=w1547:string, "error out"=w1561:errorcluster)  [unwired: 9 in]
          n561 = call <vilib>:"Get Array Elements.vi"("JSON"=w1547) -> ("<JSON>"=w1544:string[])  [unwired: 8 in, 2 out]
          n562 = Match Pattern(string=w1551, regular expression="200 OK" ("Regulärer Ausdruck")) -> (offset past match=w1552:i32)  [unwired: 1 in, 3 out]
          n563 = Search 1D Array(1D array=w1544, element=w1543) -> (index of element=w1542:i32)  [unwired: 1 in]
          n564 = Greater Than 0?(x=w1552) -> (x > 0?=w1549:bool)
          n565 = call <vilib>:"ListHeaders.vi"("client handle"=w1557, "error in (no error)"=w1561) -> ("client handle out"=w1555:T6, "headers"=w1554:string, "error out"=w1550:errorcluster)  [unwired: 11 in]
          n566 = Greater Or Equal To 0?(x=w1542) -> (x >= 0?=w1541:bool)
          n567 = Compound Arithmetic op=AND ("Mehrfacharithmetik")(invert w1550, w1549, w1541) -> (w1548:bool)
        }
        frame "Vorgang: Generate a CSV file" {
          w1568 = "Test.csv" ("String")
          # "/r/vorgang/{vNr}/{produkt}.csv"
          n568 = call <vilib>:"AddHeader.vi"("client handle"=w1599, "header"="Content-Type", "value"="text/csv", "error in (no error)"=w1600) -> ("client handle out"=w1597:T6, "error out"=w1569:errorcluster)  [unwired: 10 in]
          n569 = Concatenate Strings(w1596, "/r/vorgang/" ("String"), w1594, "/" ("String"), w1592, ".csv" ("String")) -> (w1571:string)
          n570 = control-ref of="Dieses VI"() -> (w1570:refnum<vi>)
          n571 = call "LabVIEW.Service.File_path.vi"("Fehler (Eingang, kein Fehler)"=w1569, "File name"=w1568, "VI Reference"=w1570) -> ("Fehler (Ausgang)"=w1567:errorcluster, "Dateipfad-Bedienelement"=w1566:path)  [unwired: 7 in]
          n572 = Path To String(path=w1566) -> (string=w1565:string)
          n573 = call <vilib>:"GET.vi"("client handle"=w1597, "output file"=w1566, "url"=w1571, "error in (no error)"=w1567) -> ("client handle out"=w1579:T6, "headers"=w1582:string, "body"=w1588:string, "error out"=w1576:errorcluster)  [unwired: 8 in]
          n574 = call "LabVIEW.HTTPs_Client.Handle_File.vi"("Command"=T5."read csv", "Fehler (Eingang, kein Fehler)"=w1576, "File name"=w1568, "SN"=w1573) -> ("Fehler (Ausgang)"=w1575:errorcluster, "Successful?"=w1574:bool)  [unwired: 6 in]
          n575 = call <vilib>:"AddHeader.vi"("client handle"=w1579, "header"="Content-Type", "value"="application/json", "error in (no error)"=w1575) -> ("client handle out"=w1578:T6, "error out"=w1577:errorcluster)  [unwired: 10 in]
          n576 = Match Pattern(string=w1582, regular expression="200 OK" ("Regulärer Ausdruck")) -> (offset past match=w1586:i32)  [unwired: 1 in, 3 out]
          n577 = call <vilib>:"ListHeaders.vi"("client handle"=w1578, "error in (no error)"=w1577) -> ("client handle out"=w1590:T6, "headers"=w1589:string, "error out"=w1584:errorcluster)  [unwired: 11 in]
          n578 = Greater Than 0?(x=w1586) -> (x > 0?=w1585:bool)
          n579 = Compound Arithmetic op=AND ("Mehrfacharithmetik")(invert w1584, w1585, w1574) -> (w1583:bool)
        }
        frame "Vorgang: Generate an XLSX file" {
          w1605 = "Test.xlsx" ("String")
          # "/r/vorgang/{vNr}/{produkt}.xlsx"
          n580 = call <vilib>:"AddHeader.vi"("client handle"=w1637, "header"="Content-Type", "value"="application/vnd.openxmlformats-officedocument.spreadsheetml.sheet", "error in (no error)"=w1638) -> ("client handle out"=w1635:T6, "error out"=w1608:errorcluster)  [unwired: 10 in]
          n581 = Concatenate Strings(w1634, "/r/vorgang/" ("String"), w1632, "/" ("String"), w1630, ".xlsx" ("String")) -> (w1609:string)
          n582 = control-ref of="Dieses VI"() -> (w1606:refnum<vi>)
          n583 = call "LabVIEW.Service.File_path.vi"("Fehler (Eingang, kein Fehler)"=w1608, "File name"=w1605, "VI Reference"=w1606) -> ("Fehler (Ausgang)"=w1607:errorcluster, "Dateipfad-Bedienelement"=w1604:path)  [unwired: 7 in]
          n584 = Path To String(path=w1604) -> (string=w1603:string)
          n585 = call <vilib>:"GET.vi"("client handle"=w1635, "output file"=w1604, "url"=w1609, "error in (no error)"=w1607) -> ("client handle out"=w1617:T6, "headers"=w1620:string, "body"=w1626:string, "error out"=w1614:errorcluster)  [unwired: 8 in]
          n586 = call "LabVIEW.HTTPs_Client.Handle_File.vi"("Command"=T5."read xlsx", "Fehler (Eingang, kein Fehler)"=w1614, "File name"=w1605, "SN"=w1611) -> ("Fehler (Ausgang)"=w1613:errorcluster, "Successful?"=w1612:bool)  [unwired: 6 in]
          n587 = call <vilib>:"AddHeader.vi"("client handle"=w1617, "header"="Content-Type", "value"="application/json", "error in (no error)"=w1613) -> ("client handle out"=w1616:T6, "error out"=w1615:errorcluster)  [unwired: 10 in]
          n588 = Match Pattern(string=w1620, regular expression="200 OK" ("Regulärer Ausdruck")) -> (offset past match=w1624:i32)  [unwired: 1 in, 3 out]
          n589 = call <vilib>:"ListHeaders.vi"("client handle"=w1616, "error in (no error)"=w1615) -> ("client handle out"=w1628:T6, "headers"=w1627:string, "error out"=w1622:errorcluster)  [unwired: 11 in]
          n590 = Greater Than 0?(x=w1624) -> (x > 0?=w1623:bool)
          n591 = Compound Arithmetic op=AND ("Mehrfacharithmetik")(invert w1622, w1623, w1612) -> (w1621:bool)
        }
        frame "Vorgang: Get a CSV file(Fertigmeldung report)" {
          w1648 = TRUE ("Alle ersetzen? (F)")
          # "/r/vorgang/{vNr}/csv/{fileName}"
          n592 = call "LabVIEW.FGV.Store_ID.vi"("Command"=enum16{"clear", "write", "read"}."read", "error in (no error)"=w1658) -> ("Fertigmeldung out[]"=w1657:string[], "error out"=w1645:errorcluster)  [unwired: 8 in, 4 out]
          n593 = Index Array(array=w1657, index=2 ("Index")) -> (element=w1643:string)
          n594 = Search and Replace String(replace all?=w1648, case sensitive?=w1648, input string=w1643, search string="\"" ("Such-String"), replace string="", error in=w1645) -> (result string=w1642:string, error out=w1644:errorcluster)  [unwired: 2 in, 2 out]
          n595 = Concatenate Strings(w1672, "/r/vorgang/" ("String"), w1651, "/csv/" ("String"), w1642) -> (w1641:string)
          n596 = call <vilib>:"GET.vi"("client handle"=w1671, "url"=w1641, "error in (no error)"=w1644) -> ("client handle out"=w1668:T6, "headers"=w1660:string, "body"=w1652:string, "error out"=w1666:errorcluster)  [unwired: 9 in]
          n597 = call <vilib>:"ListHeaders.vi"("client handle"=w1668, "error in (no error)"=w1666) -> ("client handle out"=w1669:T6, "headers"=w1667:string, "error out"=w1663:errorcluster)  [unwired: 11 in]
          n598 = Match Pattern(string=w1660, regular expression="200 OK" ("Regulärer Ausdruck")) -> (offset past match=w1664:i32)  [unwired: 1 in, 3 out]
          n599 = Match Pattern(string=w1652, regular expression=w1654) -> (offset past match=w1655:i32)  [unwired: 1 in, 3 out]
          n600 = Match Pattern(string=w1652, regular expression=w1651) -> (offset past match=w1653:i32)  [unwired: 1 in, 3 out]
          n601 = Greater Than 0?(x=w1664) -> (x > 0?=w1661:bool)
          n602 = Greater Than 0?(x=w1655) -> (x > 0?=w1650:bool)
          n603 = Greater Than 0?(x=w1653) -> (x > 0?=w1649:bool)
          n604 = Compound Arithmetic op=AND ("Mehrfacharithmetik")(invert w1663, w1661, w1650, w1649) -> (w1662:bool)
        }
        frame "Fertigmeldung: Create a Fertigmeldung" {
          w1694 = "\"" ("String")
          w1696 = "\"" ("String")
          w1698 = "\"" ("String")
          # "/r/fertigmeldung"
          n605 = Concatenate Strings(w1698, w1697, w1698) -> (w1691:string)
          n606 = Concatenate Strings(w1694, w1693, w1694) -> (w1692:string)
          n607 = Concatenate Strings(w1696, w1695, w1696) -> (w1690:string)
          n608 = Build Array(w1692) -> (w1689:string[])
          n609 = call "LabVIEW.Service.JSON_Input.vi"("Value 4"="\"\"", "Value 3"="false", "Command"=LabVIEW.Service.JSON_Input_Command."Fertigmeldung Create/Revert a Fertigmeldung", "Fehler (Eingang, kein Fehler)"=w1701, "Value[]"=w1689, "Value 1"=w1691, "Value 2"=w1690) -> ("Fehler (Ausgang)"=w1706:errorcluster, "<JSON>"=w1675:string)  [unwired: 3 in]
          n610 = Concatenate Strings(w1678, "/r/fertigmeldung") -> (w1676:string)
          n611 = call-poly <vilib>:"POST.vi"("client handle"=w1704, "url"=w1676, "buffer"=w1675, "error in (no error)"=w1706) -> ("client handle out"=w1702:T6, "headers"=w1679:string, "body"=w1685:string, "error out"=w1686:errorcluster)  [unwired: 8 in]
          n612 = call <vilib>:"ListHeaders.vi"("client handle"=w1702, "error in (no error)"=w1686) -> ("client handle out"=w1703:T6, "headers"=w1699:string, "error out"=w1680:errorcluster)  [unwired: 11 in]
          n613 = Match Pattern(string=w1679, regular expression="201" ("Regulärer Ausdruck")) -> (offset past match=w1683:i32)  [unwired: 1 in, 3 out]
          n614 = Greater Than 0?(x=w1683) -> (x > 0?=w1682:bool)
          n615 = Compound Arithmetic op=AND ("Mehrfacharithmetik")(invert w1680, w1682) -> (w1681:bool)
        }
        frame "Fertigmeldung: Revert the Fertigmeldung" {
          w1726 = "\"" ("String")
          w1728 = "\"" ("String")
          w1730 = "\"" ("String")
          # "/r/fertigmeldung/revert"
          n616 = Concatenate Strings(w1730, w1729, w1730) -> (w1723:string)
          n617 = Concatenate Strings(w1726, w1725, w1726) -> (w1724:string)
          n618 = Concatenate Strings(w1728, w1727, w1728) -> (w1722:string)
          n619 = Build Array(w1724) -> (w1721:string[])
          n620 = call "LabVIEW.Service.JSON_Input.vi"("Value 4"="\"\"", "Value 3"="false", "Command"=LabVIEW.Service.JSON_Input_Command."Fertigmeldung Create/Revert a Fertigmeldung", "Fehler (Eingang, kein Fehler)"=w1733, "Value[]"=w1721, "Value 1"=w1723, "Value 2"=w1722) -> ("Fehler (Ausgang)"=w1738:errorcluster, "<JSON>"=w1707:string)  [unwired: 3 in]
          n621 = Concatenate Strings(w1710, "/r/fertigmeldung/revert") -> (w1708:string)
          n622 = call-poly <vilib>:"POST.vi"("client handle"=w1736, "url"=w1708, "buffer"=w1707, "error in (no error)"=w1738) -> ("client handle out"=w1734:T6, "headers"=w1711:string, "body"=w1717:string, "error out"=w1718:errorcluster)  [unwired: 8 in]
          n623 = call <vilib>:"ListHeaders.vi"("client handle"=w1734, "error in (no error)"=w1718) -> ("client handle out"=w1735:T6, "headers"=w1731:string, "error out"=w1712:errorcluster)  [unwired: 11 in]
          n624 = Match Pattern(string=w1711, regular expression="201" ("Regulärer Ausdruck")) -> (offset past match=w1715:i32)  [unwired: 1 in, 3 out]
          n625 = Greater Than 0?(x=w1715) -> (x > 0?=w1714:bool)
          n626 = Compound Arithmetic op=AND ("Mehrfacharithmetik")(invert w1712, w1714) -> (w1713:bool)
        }
        frame "User: Get all users" {
          # "/r/personen"
          n627 = Concatenate Strings(w1766, "/r/personen") -> (w1739:string)
          n628 = call <vilib>:"GET.vi"("client handle"=w1771, "url"=w1739, "error in (no error)"=w1772) -> ("client handle out"=w1767:T6, "headers"=w1761:string, "body"=w1742:string, "error out"=w1759:errorcluster)  [unwired: 9 in]
          n629 = call <vilib>:"Find Multiple Items.vi"("$Path or Item Name"="$[*].username", "error in (no error)"=w1759, "JSON"=w1742) -> ("error out"=w1754:errorcluster, "<JSON>"=w1757:string[])  [unwired: 5 in, 2 out]
          n630 = Search 1D Array(1D array=w1757, element="\"test\"" ("Element")) -> (index of element=w1741:i32)  [unwired: 1 in]
          n631 = call <vilib>:"Find Multiple Items.vi"("$Path or Item Name"="$[*].id", "error in (no error)"=w1754, "JSON"=w1742) -> ("error out"=w1751:errorcluster, "<JSON>"=w1753:string[])  [unwired: 5 in, 2 out]
          n632 = Index Array(array=w1753, index=w1741) -> (element=w1750:string)
          n633 = call "LabVIEW.FGV.Store_ID.vi"("ID In"=w1750, "Command"=enum16{"clear", "write", "read"}."write", "error in (no error)"=w1751) -> ("error out"=w1748:errorcluster)  [unwired: 7 in, 5 out]
          n634 = call <vilib>:"Find Multiple Items.vi"("$Path or Item Name"="$[*].roles", "error in (no error)"=w1748, "JSON"=w1742) -> ("error out"=w1740:errorcluster, "<JSON>"=w1747:string[])  [unwired: 5 in, 2 out]
          n635 = Index Array(array=w1747, index=w1741) -> (element=w1744:string)
          n636 = Match Pattern(string=w1744, regular expression="API Test" ("Regulärer Ausdruck")) -> (offset past match=w1746:i32)  [unwired: 1 in, 3 out]
          n637 = Match Pattern(string=w1761, regular expression="200 OK" ("Regulärer Ausdruck")) -> (offset past match=w1764:i32)  [unwired: 1 in, 3 out]
          n638 = call <vilib>:"ListHeaders.vi"("client handle"=w1767, "error in (no error)"=w1740) -> ("client handle out"=w1770:T6, "headers"=w1768:string, "error out"=w1762:errorcluster)  [unwired: 11 in]
          n639 = Greater Than 0?(x=w1746) -> (x > 0?=w1743:bool)
          n640 = Greater Than 0?(x=w1764) -> (x > 0?=w1763:bool)
          n641 = Compound Arithmetic op=AND ("Mehrfacharithmetik")(invert w1762, w1763, w1743) -> (w1758:bool)
        }
        frame "User: Update an user" {
          # "/r/personen/{id}"
          n642 = call "LabVIEW.FGV.Store_ID.vi"("Command"=enum16{"clear", "write", "read"}."read", "error in (no error)"=w1797) -> ("ID Out"=w1783:string, "File Name Out"=w1782:string, "error out"=w1796:errorcluster)  [unwired: 8 in, 3 out]
          n643 = Build Array(w1782) -> (w1781:string[])
          n644 = Concatenate Strings(w1799, "/r/personen/", w1783) -> (w1775:string)
          n645 = call "LabVIEW.Service.JSON_Input.vi"("Command"=LabVIEW.Service.JSON_Input_Command."User Update a user", "Fehler (Eingang, kein Fehler)"=w1796, "Value[]"=w1781, "Value 1"=w1777) -> ("Fehler (Ausgang)"=w1806:errorcluster, "<JSON>"=w1774:string)  [unwired: 6 in]
          n646 = Equal?(x=w1777, y="null") -> (x = y?=w1779:bool)
          n647 = call-poly <vilib>:"PUT.vi"("client handle"=w1804, "url"=w1775, "buffer"=w1774, "error in (no error)"=w1806) -> ("client handle out"=w1803:T6, "headers"=w1787:string, "body"=w1792:string, "error out"=w1794:errorcluster)  [unwired: 8 in]
          n648 = Select(t="\"\"" ("y"), s=w1779, f=w1777) -> (s? t:f=w1776:string)
          n649 = call <vilib>:"Find Item.vi"("$Path or Item Name"="infoText", "error in (no error)"=w1794, "JSON"=w1792) -> ("error out"=w1793:errorcluster, "<JSON>"=w1786:string)  [unwired: 5 in, 2 out]
          n650 = call <vilib>:"ListHeaders.vi"("client handle"=w1803, "error in (no error)"=w1793) -> ("client handle out"=w1801:T6, "headers"=w1800:string, "error out"=w1788:errorcluster)  [unwired: 11 in]
          n651 = Equal?(x=w1786, y=w1776) -> (x = y?=w1785:bool)
          n652 = Match Pattern(string=w1787, regular expression="200 OK" ("Regulärer Ausdruck")) -> (offset past match=w1790:i32)  [unwired: 1 in, 3 out]
          n653 = Greater Than 0?(x=w1790) -> (x > 0?=w1789:bool)
          n654 = Compound Arithmetic op=AND ("Mehrfacharithmetik")(invert w1788, w1789, w1785) -> (w1784:bool)
        }
        frame "User: Get a single user" {
          # "/r/personen/{id}"
          n655 = call "LabVIEW.FGV.Store_ID.vi"("Command"=enum16{"clear", "write", "read"}."read", "error in (no error)"=w1835) -> ("ID Out"=w1832:string, "error out"=w1833:errorcluster)  [unwired: 8 in, 4 out]
          n656 = Concatenate Strings(w1809, "/r/personen/", w1832) -> (w1808:string)
          n657 = call <vilib>:"GET.vi"("client handle"=w1834, "url"=w1808, "error in (no error)"=w1833) -> ("client handle out"=w1830:T6, "headers"=w1823:string, "body"=w1812:string, "error out"=w1820:errorcluster)  [unwired: 9 in]
          n658 = call <vilib>:"Find Item.vi"("$Path or Item Name"="infoText", "error in (no error)"=w1820, "JSON"=w1812) -> ("error out"=w1816:errorcluster, "<JSON>"=w1819:string)  [unwired: 5 in, 2 out]
          n659 = call <vilib>:"Find Item.vi"("$Path or Item Name"="username", "error in (no error)"=w1816, "JSON"=w1812) -> ("error out"=w1815:errorcluster, "<JSON>"=w1814:string)  [unwired: 5 in, 2 out]
          n660 = Match Pattern(string=w1823, regular expression="200 OK" ("Regulärer Ausdruck")) -> (offset past match=w1827:i32)  [unwired: 1 in, 3 out]
          n661 = call <vilib>:"ListHeaders.vi"("client handle"=w1830, "error in (no error)"=w1815) -> ("client handle out"=w1831:T6, "headers"=w1824:string, "error out"=w1825:errorcluster)  [unwired: 11 in]
          n662 = Equal?(x=w1819, y=w1818) -> (x = y?=w1810:bool)
          n663 = Greater Than 0?(x=w1827) -> (x > 0?=w1826:bool)
          n664 = Equal?(x=w1814, y="\"test\"") -> (x = y?=w1811:bool)
          n665 = Compound Arithmetic op=AND ("Mehrfacharithmetik")(invert w1825, w1826, w1811) -> (w1822:bool)
        }
        frame "User: Get all user roles" {
          # "/r/roles"
          n666 = Concatenate Strings(w1864, "/r/roles") -> (w1838:string)
          n667 = call <vilib>:"GET.vi"("client handle"=w1869, "url"=w1838, "error in (no error)"=w1866) -> ("client handle out"=w1868:T6, "headers"=w1856:string, "body"=w1848:string, "error out"=w1854:errorcluster)  [unwired: 9 in]
          n668 = call <vilib>:"Find Multiple Items.vi"("$Path or Item Name"="$[*].name", "error in (no error)"=w1854, "JSON"=w1848) -> ("error out"=w1852:errorcluster, "<JSON>"=w1851:string[])  [unwired: 5 in, 2 out]
          n669 = call <vilib>:"Find Multiple Items.vi"("$Path or Item Name"="$[*].id", "error in (no error)"=w1852, "JSON"=w1848) -> ("error out"=w1844:errorcluster, "<JSON>"=w1847:string[])  [unwired: 5 in, 2 out]
          n670 = Search 1D Array(1D array=w1851, element="\"API Test\"" ("Element")) -> (index of element=w1846:i32)  [unwired: 1 in]
          n671 = Index Array(array=w1847, index=w1846) -> (element=w1839:string)
          n672 = call "LabVIEW.FGV.Store_ID.vi"("Command"=enum16{"clear", "write", "read"}."read", "error in (no error)"=w1844) -> ("ID Out"=w1840:string, "error out"=w1842:errorcluster)  [unwired: 8 in, 4 out]
          n673 = call "LabVIEW.FGV.Store_ID.vi"("ID In"=w1840, "Command"=enum16{"clear", "write", "read"}."write", "error in (no error)"=w1842, "File Name In"=w1839) -> ("error out"=w1841:errorcluster)  [unwired: 6 in, 5 out]
          n674 = Match Pattern(string=w1856, regular expression="200 OK" ("Regulärer Ausdruck")) -> (offset past match=w1860:i32)  [unwired: 1 in, 3 out]
          n675 = call <vilib>:"ListHeaders.vi"("client handle"=w1868, "error in (no error)"=w1841) -> ("client handle out"=w1867:T6, "headers"=w1863:string, "error out"=w1857:errorcluster)  [unwired: 11 in]
          n676 = Greater Than 0?(x=w1860) -> (x > 0?=w1859:bool)
          n677 = Greater Or Equal To 0?(x=w1846) -> (x >= 0?=w1849:bool)
          n678 = Compound Arithmetic op=AND ("Mehrfacharithmetik")(invert w1857, w1859, w1849) -> (w1858:bool)
        }
        frame "User: Get a single user role" {
          # "/r/roles/{id}"
          n679 = call "LabVIEW.FGV.Store_ID.vi"("Command"=enum16{"clear", "write", "read"}."read", "error in (no error)"=w1892) -> ("ID Out"=w1871:string, "File Name Out"=w1872:string, "error out"=w1891:errorcluster)  [unwired: 8 in, 3 out]
          n680 = Concatenate Strings(w1894, "/r/roles/", w1872) -> (w1870:string)
          n681 = call <vilib>:"GET.vi"("client handle"=w1898, "url"=w1870, "error in (no error)"=w1891) -> ("client handle out"=w1897:T6, "headers"=w1885:string, "body"=w1877:string, "error out"=w1889:errorcluster)  [unwired: 9 in]
          n682 = call <vilib>:"Find Item.vi"("$Path or Item Name"="name", "error in (no error)"=w1889, "JSON"=w1877) -> ("error out"=w1878:errorcluster, "<JSON>"=w1882:string)  [unwired: 5 in, 2 out]
          n683 = call <vilib>:"Find Multiple Items.vi"("$Path or Item Name"="$.permissions[*]", "error in (no error)"=w1878, "JSON"=w1877) -> ("error out"=w1875:errorcluster, "<JSON>"=w1873:string[])  [unwired: 5 in, 2 out]
          n684 = call "LabVIEW.FGV.Store_ID.vi"("ID In"=w1871, "Command"=enum16{"clear", "write", "read"}."write", "Step IDs in[]"=w1873, "error in (no error)"=w1875, "File Name In"=w1872) -> ("error out"=w1874:errorcluster)  [unwired: 5 in, 5 out]
          n685 = Match Pattern(string=w1885, regular expression="200 OK" ("Regulärer Ausdruck")) -> (offset past match=w1887:i32)  [unwired: 1 in, 3 out]
          n686 = call <vilib>:"ListHeaders.vi"("client handle"=w1897, "error in (no error)"=w1874) -> ("client handle out"=w1896:T6, "headers"=w1895:string, "error out"=w1884:errorcluster)  [unwired: 11 in]
          n687 = Greater Than 0?(x=w1887) -> (x > 0?=w1886:bool)
          n688 = Equal?(x=w1882, y="\"API Test\"" ("Element")) -> (x = y?=w1880:bool)
          n689 = Compound Arithmetic op=AND ("Mehrfacharithmetik")(invert w1884, w1886, w1880) -> (w1883:bool)
        }
        frame "User: Update a user role" {
          # "/r/roles/{id}"
          n690 = call "LabVIEW.FGV.Store_ID.vi"("Command"=enum16{"clear", "write", "read"}."read", "error in (no error)"=w1919) -> ("Step IDs out[]"=w1917:string[], "File Name Out"=w1927:string, "error out"=w1932:errorcluster)  [unwired: 8 in, 3 out]
          n691 = case shown="True" w1912 {
            tunnel: w1917 -> [w1947 w1952]
            tunnel: [w1949 w1951] -> w1916
            frame False {
              n692 = Search 1D Array(1D array=w1947, element="\"sn_run_dispach_step\"" ("Neues Element/Teil-Array")) -> (index of element=w1946:i32)  [unwired: 1 in]
              n693 = Delete From Array(array=w1947, length=1 ("Länge"), index=w1946) -> (array with subset deleted=w1949:string[])  [unwired: 1 out]
            }
            frame True {
              n694 = Insert Into Array(array=w1952, new element="\"sn_run_dispach_step\"" ("Neues Element/Teil-Array")) -> (w1951:string[])  [unwired: 1 in]
            }
          }
          n695 = Concatenate Strings(w1918, "/r/roles/", w1927) -> (w1902:string)
          n696 = call "LabVIEW.Service.JSON_Input.vi"("Command"=LabVIEW.Service.JSON_Input_Command."User Update a user role", "Fehler (Eingang, kein Fehler)"=w1932, "Value[]"=w1916) -> ("Fehler (Ausgang)"=w1935:errorcluster, "<JSON>"=w1901:string)  [unwired: 7 in]
          n697 = call-poly <vilib>:"PUT.vi"("client handle"=w1928, "url"=w1902, "buffer"=w1901, "error in (no error)"=w1935) -> ("client handle out"=w1925:T6, "headers"=w1920:string, "body"=w1907:string, "error out"=w1914:errorcluster)  [unwired: 8 in]
          n698 = call <vilib>:"Find Multiple Items.vi"("$Path or Item Name"="$.permissions[*]", "error in (no error)"=w1914, "JSON"=w1907) -> ("error out"=w1909:errorcluster, "<JSON>"=w1913:string[])  [unwired: 5 in, 2 out]
          n699 = case shown="True" w1911 {
            tunnel: w1913 -> [w1939 w1944]
            tunnel: [w1937 w1942] -> w1906
            frame False {
              n700 = Search 1D Array(1D array=w1939, element="\"sn_run_dispach_step\"" ("Neues Element/Teil-Array")) -> (index of element=w1938:i32)  [unwired: 1 in]
              n701 = Less Than 0?(x=w1938) -> (x < 0?=w1937:bool)
            }
            frame True {
              n702 = Search 1D Array(1D array=w1944, element="\"sn_run_dispach_step\"" ("Neues Element/Teil-Array")) -> (index of element=w1943:i32)  [unwired: 1 in]
              n703 = Greater Or Equal To 0?(x=w1943) -> (x >= 0?=w1942:bool)
            }
          }
          n704 = call <vilib>:"Find Item.vi"("$Path or Item Name"="name", "error in (no error)"=w1909, "JSON"=w1907) -> ("error out"=w1908:errorcluster, "<JSON>"=w1903:string)  [unwired: 5 in, 2 out]
          n705 = Match Pattern(string=w1920, regular expression="200 OK" ("Regulärer Ausdruck")) -> (offset past match=w1930:i32)  [unwired: 1 in, 3 out]
          n706 = call <vilib>:"ListHeaders.vi"("client handle"=w1925, "error in (no error)"=w1908) -> ("client handle out"=w1924:T6, "headers"=w1923:string, "error out"=w1922:errorcluster)  [unwired: 11 in]
          n707 = Equal?(x=w1903, y="\"API Test\"" ("Element")) -> (x = y?=w1904:bool)
          n708 = Greater Than 0?(x=w1930) -> (x > 0?=w1929:bool)
          n709 = Compound Arithmetic op=AND ("Mehrfacharithmetik")(invert w1922, w1929, w1904, w1906) -> (w1921:bool)
        }
        frame "User: Get all permissions" {
          # "/r/roles/permissions_usage"
          n710 = Concatenate Strings(w1977, "/r/roles/permissions_usage") -> (w1953:string)
          n711 = call <vilib>:"GET.vi"("client handle"=w1980, "url"=w1953, "error in (no error)"=w1976) -> ("client handle out"=w1979:T6, "headers"=w1971:string, "body"=w1955:string, "error out"=w1968:errorcluster)  [unwired: 9 in]
          n712 = call <vilib>:"Find Multiple Items.vi"("$Path or Item Name"="$[*].permission", "error in (no error)"=w1968, "JSON"=w1955) -> ("error out"=w1963:errorcluster, "<JSON>"=w1967:string[])  [unwired: 5 in, 2 out]
          n713 = call <vilib>:"Find Multiple Items.vi"("$Path or Item Name"="$[*].listOfUsers", "error in (no error)"=w1963, "JSON"=w1955) -> ("error out"=w1959:errorcluster, "<JSON>"=w1962:string[])  [unwired: 5 in, 2 out]
          n714 = Search 1D Array(1D array=w1967, element="\"sn_run_dispach_step\"" ("Regulärer Ausdruck")) -> (index of element=w1961:i32)  [unwired: 1 in]
          n715 = Index Array(array=w1962, index=w1961) -> (element=w1960:string)
          n716 = call <vilib>:"Get Array Elements.vi"("error in (no error)"=w1959, "JSON"=w1960) -> ("error out"=w1958:errorcluster, "<JSON>"=w1957:string[])  [unwired: 7 in, 1 out]
          n717 = case shown="True" w1956 {
            tunnel: w1957 -> [w1984 w1991]
            tunnel: [w1985 w1988] -> w1954
            frame False {
              n718 = Search 1D Array(1D array=w1984, element="\"test\"" ("Element")) -> (index of element=w1986:i32)  [unwired: 1 in]
              n719 = Less Than 0?(x=w1986) -> (x < 0?=w1985:bool)
            }
            frame True {
              n720 = Search 1D Array(1D array=w1991, element="\"test\"" ("Element")) -> (index of element=w1989:i32)  [unwired: 1 in]
              n721 = Greater Or Equal To 0?(x=w1989) -> (x >= 0?=w1988:bool)
            }
          }
          n722 = call <vilib>:"ListHeaders.vi"("client handle"=w1979, "error in (no error)"=w1958) -> ("client handle out"=w1982:T6, "headers"=w1981:string, "error out"=w1972:errorcluster)  [unwired: 11 in]
          n723 = Match Pattern(string=w1971, regular expression="200 OK" ("Regulärer Ausdruck")) -> (offset past match=w1974:i32)  [unwired: 1 in, 3 out]
          n724 = Greater Than 0?(x=w1974) -> (x > 0?=w1973:bool)
          n725 = Greater Or Equal To 0?(x=w1961) -> (x >= 0?=w1965:bool)
          n726 = Compound Arithmetic op=AND ("Mehrfacharithmetik")(invert w1972, w1973, w1965) -> (w1970:bool)
        }
        frame "Search: Get Vorgang/Produkt combinations" {
          w1999 = "\"" ("String")
          # "/r/search/vorgang_produkt"
          n727 = Concatenate Strings(w2020, "/r/search/vorgang_produkt" ("String"), "?searchTerm=" ("String"), w1998) -> (w1992:string)
          n728 = call <vilib>:"GET.vi"("client handle"=w2022, "url"=w1992, "error in (no error)"=w2021) -> ("client handle out"=w2017:T6, "headers"=w2013:string, "body"=w2005:string, "error out"=w2007:errorcluster)  [unwired: 9 in]
          n729 = call <vilib>:"Find Multiple Items.vi"("$Path or Item Name"="$.results[*].resultType", "error in (no error)"=w2007, "JSON"=w2005) -> ("error out"=w2008:errorcluster, "<JSON>"=w2004:string[])  [unwired: 5 in, 2 out]
          n730 = call <vilib>:"Find Multiple Items.vi"("$Path or Item Name"="$.results[*].vorgangsnummer", "error in (no error)"=w2008, "JSON"=w2005) -> ("error out"=w2006:errorcluster, "<JSON>"=w1995:string[])  [unwired: 5 in, 2 out]
          n731 = Index Array(array=w2004, index=0 ("Index")) -> (element=w2002:string)
          n732 = Match Pattern(string=w2013, regular expression="200 OK" ("Regulärer Ausdruck")) -> (offset past match=w2024:i32)  [unwired: 1 in, 3 out]
          n733 = Index Array(array=w1995, index=0 ("Index")) -> (element=w1994:string)
          n734 = Concatenate Strings(w1999, w1998, w1999) -> (w1997:string)
          n735 = Greater Than 0?(x=w2024) -> (x > 0?=w2023:bool)
          n736 = Equal?(x=w2002, y="\"vorgang\"") -> (x = y?=w2000:bool)
          n737 = Equal?(x=w1994, y=w1997) -> (x = y?=w1993:bool)
          n738 = call <vilib>:"ListHeaders.vi"("client handle"=w2017, "error in (no error)"=w2006) -> ("client handle out"=w2016:T6, "headers"=w2014:string, "error out"=w2011:errorcluster)  [unwired: 11 in]
          n739 = Compound Arithmetic op=AND ("Mehrfacharithmetik")(invert w2011, w2023, w2000, w1993) -> (w2012:bool)
        }
        frame "Search: Get Vorgang/Produkt/SN combinations" {
          w2034 = "\"" ("String")
          # "/r/search/vorgang_produkt_seriennummer"
          n740 = Concatenate Strings(w2054, "/r/search/vorgang_produkt_seriennummer" ("String"), "?searchTerm=" ("String"), w2033) -> (w2026:string)
          n741 = call <vilib>:"GET.vi"("client handle"=w2056, "url"=w2026, "error in (no error)"=w2055) -> ("client handle out"=w2051:T6, "headers"=w2047:string, "body"=w2032:string, "error out"=w2043:errorcluster)  [unwired: 9 in]
          n742 = call <vilib>:"Find Multiple Items.vi"("$Path or Item Name"="$.results[*].resultType", "error in (no error)"=w2043, "JSON"=w2032) -> ("error out"=w2036:errorcluster, "<JSON>"=w2042:string[])  [unwired: 5 in, 2 out]
          n743 = call <vilib>:"Find Multiple Items.vi"("$Path or Item Name"="$.results[*].seriennummer", "error in (no error)"=w2036, "JSON"=w2032) -> ("error out"=w2035:errorcluster, "<JSON>"=w2029:string[])  [unwired: 5 in, 2 out]
          n744 = Index Array(array=w2042, index=0 ("Index")) -> (element=w2040:string)
          n745 = Match Pattern(string=w2047, regular expression="200 OK" ("Regulärer Ausdruck")) -> (offset past match=w2058:i32)  [unwired: 1 in, 3 out]
          n746 = Index Array(array=w2029, index=0 ("Index")) -> (element=w2030:string)
          n747 = Concatenate Strings(w2034, w2033, w2034) -> (w2028:string)
          n748 = Greater Than 0?(x=w2058) -> (x > 0?=w2057:bool)
          n749 = call <vilib>:"ListHeaders.vi"("client handle"=w2051, "error in (no error)"=w2035) -> ("client handle out"=w2050:T6, "headers"=w2048:string, "error out"=w2045:errorcluster)  [unwired: 11 in]
          n750 = Equal?(x=w2030, y=w2028) -> (x = y?=w2027:bool)
          n751 = Equal?(x=w2040, y="\"seriennummer\"") -> (x = y?=w2038:bool)
          n752 = Compound Arithmetic op=AND ("Mehrfacharithmetik")(invert w2045, w2057, w2038, w2027) -> (w2046:bool)
        }
        frame "Search: Get Seriennummern by Vorgang and Produkt" {
          w2067 = "\"" ("String")
          # "/r/search/seriennummern_by_vorgang_produkt"
          n753 = Concatenate Strings(w2083, "/r/search/seriennummern_by_vorgang_produkt" ("String"), "?vorgangsnummer=" ("String"), w2073, "&produktname=" ("String"), w2071) -> (w2060:string)
          n754 = call <vilib>:"GET.vi"("client handle"=w2085, "url"=w2060, "error in (no error)"=w2084) -> ("client handle out"=w2080:T6, "headers"=w2076:string, "body"=w2064:string, "error out"=w2069:errorcluster)  [unwired: 9 in]
          n755 = call <vilib>:"Find Multiple Items.vi"("$Path or Item Name"="$.results[*].sn", "error in (no error)"=w2069, "JSON"=w2064) -> ("error out"=w2068:errorcluster, "<JSON>"=w2062:string[])  [unwired: 5 in, 2 out]
          n756 = Concatenate Strings(w2067, w2066, w2067) -> (w2065:string)
          n757 = Search 1D Array(1D array=w2062, element=w2065) -> (index of element=w2063:i32)  [unwired: 1 in]
          n758 = Match Pattern(string=w2076, regular expression="200 OK" ("Regulärer Ausdruck")) -> (offset past match=w2087:i32)  [unwired: 1 in, 3 out]
          n759 = Greater Than 0?(x=w2087) -> (x > 0?=w2086:bool)
          n760 = Greater Or Equal To 0?(x=w2063) -> (x >= 0?=w2061:bool)
          n761 = call <vilib>:"ListHeaders.vi"("client handle"=w2080, "error in (no error)"=w2068) -> ("client handle out"=w2079:T6, "headers"=w2077:string, "error out"=w2074:errorcluster)  [unwired: 11 in]
          n762 = Compound Arithmetic op=AND ("Mehrfacharithmetik")(invert w2074, w2086, w2061) -> (w2075:bool)
        }
        frame "Search: Lookup Vorgang" {
          w2096 = "\"" ("String")
          # "/r/search/vorgang"
          n763 = Concatenate Strings(w2110, "/r/search/vorgang" ("String"), "?searchTerm=" ("String"), w2095) -> (w2089:string)
          n764 = call <vilib>:"GET.vi"("client handle"=w2112, "url"=w2089, "error in (no error)"=w2111) -> ("client handle out"=w2107:T6, "headers"=w2103:string, "body"=w2097:string, "error out"=w2099:errorcluster)  [unwired: 9 in]
          n765 = call <vilib>:"Find Multiple Items.vi"("$Path or Item Name"="$.results[*].vNr", "error in (no error)"=w2099, "JSON"=w2097) -> ("error out"=w2098:errorcluster, "<JSON>"=w2094:string[])  [unwired: 5 in, 2 out]
          n766 = Concatenate Strings(w2096, w2095, w2096) -> (w2091:string)
          n767 = Index Array(array=w2094, index=0 ("Index")) -> (element=w2092:string)
          n768 = Match Pattern(string=w2103, regular expression="200 OK" ("Regulärer Ausdruck")) -> (offset past match=w2114:i32)  [unwired: 1 in, 3 out]
          n769 = Greater Than 0?(x=w2114) -> (x > 0?=w2113:bool)
          n770 = Equal?(x=w2092, y=w2091) -> (x = y?=w2090:bool)
          n771 = call <vilib>:"ListHeaders.vi"("client handle"=w2107, "error in (no error)"=w2098) -> ("client handle out"=w2106:T6, "headers"=w2104:string, "error out"=w2101:errorcluster)  [unwired: 11 in]
          n772 = Compound Arithmetic op=AND ("Mehrfacharithmetik")(invert w2101, w2113, w2090) -> (w2102:bool)
        }
        frame "Search: Find production plan" {
          w2123 = "PP0215a-R01-0001" ("String")
          w2127 = "\"" ("String")
          # "/r/search/vorgang"
          n773 = Concatenate Strings(w2137, "/r/search/production_plan" ("String"), "?searchTerm=" ("String"), w2123) -> (w2124:string)
          n774 = call <vilib>:"GET.vi"("client handle"=w2139, "url"=w2124, "error in (no error)"=w2138) -> ("client handle out"=w2134:T6, "headers"=w2130:string, "body"=w2120:string, "error out"=w2121:errorcluster)  [unwired: 9 in]
          n775 = call <vilib>:"Find Multiple Items.vi"("$Path or Item Name"="$.results[*].productionPlanID", "error in (no error)"=w2121, "JSON"=w2120) -> ("error out"=w2119:errorcluster, "<JSON>"=w2116:string[])  [unwired: 5 in, 2 out]
          n776 = Index Array(array=w2116, index=0 ("Index")) -> (element=w2117:string)
          n777 = Concatenate Strings(w2127, w2123, w2127) -> (w2126:string)
          n778 = Match Pattern(string=w2130, regular expression="200" ("Regulärer Ausdruck")) -> (offset past match=w2141:i32)  [unwired: 1 in, 3 out]
          n779 = Greater Than 0?(x=w2141) -> (x > 0?=w2140:bool)
          n780 = Equal?(x=w2117, y=w2126) -> (x = y?=w2125:bool)
          n781 = call <vilib>:"ListHeaders.vi"("client handle"=w2134, "error in (no error)"=w2119) -> ("client handle out"=w2133:T6, "headers"=w2131:string, "error out"=w2128:errorcluster)  [unwired: 11 in]
          n782 = Compound Arithmetic op=AND ("Mehrfacharithmetik")(invert w2128, w2140, w2125) -> (w2129:bool)
        }
        frame "Search: Find production plan arrangement" {
          w2150 = "PA0215a-R01-0001" ("String")
          w2154 = "\"" ("String")
          # "/r/search/vorgang"
          n783 = Concatenate Strings(w2164, "/r/search/production_plan_arrangement" ("String"), "?searchTerm=" ("String"), w2150) -> (w2151:string)
          n784 = call <vilib>:"GET.vi"("client handle"=w2166, "url"=w2151, "error in (no error)"=w2165) -> ("client handle out"=w2161:T6, "headers"=w2157:string, "body"=w2147:string, "error out"=w2148:errorcluster)  [unwired: 9 in]
          n785 = call <vilib>:"Find Multiple Items.vi"("$Path or Item Name"="$.results[*].arrangementID", "error in (no error)"=w2148, "JSON"=w2147) -> ("error out"=w2146:errorcluster, "<JSON>"=w2143:string[])  [unwired: 5 in, 2 out]
          n786 = Index Array(array=w2143, index=0 ("Index")) -> (element=w2144:string)
          n787 = Concatenate Strings(w2154, w2150, w2154) -> (w2153:string)
          n788 = Match Pattern(string=w2157, regular expression="200" ("Regulärer Ausdruck")) -> (offset past match=w2168:i32)  [unwired: 1 in, 3 out]
          n789 = Greater Than 0?(x=w2168) -> (x > 0?=w2167:bool)
          n790 = Equal?(x=w2144, y=w2153) -> (x = y?=w2152:bool)
          n791 = call <vilib>:"ListHeaders.vi"("client handle"=w2161, "error in (no error)"=w2146) -> ("client handle out"=w2160:T6, "headers"=w2158:string, "error out"=w2155:errorcluster)  [unwired: 11 in]
          n792 = Compound Arithmetic op=AND ("Mehrfacharithmetik")(invert w2155, w2167, w2152) -> (w2156:bool)
        }
        frame "MAC addresses: Get all reserved MAC addresses" {
          w2173 = "\"" ("String")
          # "/r/mac_address_auto/seriennummer/{seriennummer}"
          n793 = Concatenate Strings(w2188, "/r/mac_address_auto/seriennummer/" ("String"), w2187) -> (w2170:string)
          n794 = call <vilib>:"GET.vi"("client handle"=w2192, "url"=w2170, "error in (no error)"=w2194) -> ("client handle out"=w2191:T6, "headers"=w2184:string, "body"=w2178:string, "error out"=w2180:errorcluster)  [unwired: 9 in]
          n795 = call <vilib>:"Find Multiple Items.vi"("$Path or Item Name"="$[*].address", "error in (no error)"=w2180, "JSON"=w2178) -> ("error out"=w2179:errorcluster, "<JSON>"=w2177:string[])  [unwired: 5 in, 2 out]
          n796 = Concatenate Strings(w2173, w2172, w2173) -> (w2171:string)
          n797 = Search 1D Array(1D array=w2177, element=w2171) -> (index of element=w2176:i32)  [unwired: 1 in]
          n798 = Match Pattern(string=w2184, regular expression="200 OK" ("Regulärer Ausdruck")) -> (offset past match=w2185:i32)  [unwired: 1 in, 3 out]
          n799 = call <vilib>:"ListHeaders.vi"("client handle"=w2191, "error in (no error)"=w2179) -> ("client handle out"=w2190:T6, "headers"=w2189:string, "error out"=w2183:errorcluster)  [unwired: 11 in]
          n800 = Greater Than 0?(x=w2185) -> (x > 0?=w2182:bool)
          n801 = Greater Or Equal To 0?(x=w2176) -> (x >= 0?=w2175:bool)
          n802 = Compound Arithmetic op=AND ("Mehrfacharithmetik")(invert w2183, w2182, w2175) -> (w2174:bool)
        }
        frame "MAC addresses: Get the most recently reserved MAC addresses" {
          w2199 = "\"" ("String")
          # "/r/mac_address_auto/seriennummer/{seriennummer}/most_recent_reservation"
          n803 = Concatenate Strings(w2215, "/r/mac_address_auto/seriennummer/" ("String"), w2214, "/most_recent_reservation" ("String")) -> (w2196:string)
          n804 = call <vilib>:"GET.vi"("client handle"=w2219, "url"=w2196, "error in (no error)"=w2221) -> ("client handle out"=w2218:T6, "headers"=w2211:string, "body"=w2205:string, "error out"=w2207:errorcluster)  [unwired: 9 in]
          n805 = call <vilib>:"Find Multiple Items.vi"("$Path or Item Name"="$[*].address", "error in (no error)"=w2207, "JSON"=w2205) -> ("error out"=w2206:errorcluster, "<JSON>"=w2204:string[])  [unwired: 5 in, 2 out]
          n806 = Concatenate Strings(w2199, w2197, w2199) -> (w2198:string)
          n807 = Search 1D Array(1D array=w2204, element=w2198) -> (index of element=w2203:i32)  [unwired: 1 in]
          n808 = Match Pattern(string=w2211, regular expression="200 OK" ("Regulärer Ausdruck")) -> (offset past match=w2212:i32)  [unwired: 1 in, 3 out]
          n809 = call <vilib>:"ListHeaders.vi"("client handle"=w2218, "error in (no error)"=w2206) -> ("client handle out"=w2217:T6, "headers"=w2216:string, "error out"=w2210:errorcluster)  [unwired: 11 in]
          n810 = Greater Than 0?(x=w2212) -> (x > 0?=w2209:bool)
          n811 = Greater Or Equal To 0?(x=w2203) -> (x >= 0?=w2202:bool)
          n812 = Compound Arithmetic op=AND ("Mehrfacharithmetik")(invert w2210, w2209, w2202) -> (w2201:bool)
        }
        frame "MAC addresses: Get data for a MAC address" {
          w2227 = "\"" ("String")
          # "/r/mac_address_auto/address/{macAddress}"
          n813 = Concatenate Strings(w2240, "/r/mac_address_auto/address/" ("String"), w2224) -> (w2223:string)
          n814 = call <vilib>:"GET.vi"("client handle"=w2244, "url"=w2223, "error in (no error)"=w2246) -> ("client handle out"=w2243:T6, "headers"=w2237:string, "body"=w2230:string, "error out"=w2232:errorcluster)  [unwired: 9 in]
          n815 = Concatenate Strings(w2227, w2225, w2227) -> (w2226:string)
          n816 = call <vilib>:"Find Item.vi"("$Path or Item Name"="serialNumber", "error in (no error)"=w2232, "JSON"=w2230) -> ("error out"=w2231:errorcluster, "<JSON>"=w2229:string)  [unwired: 5 in, 2 out]
          n817 = Match Pattern(string=w2237, regular expression="200 OK" ("Regulärer Ausdruck")) -> (offset past match=w2238:i32)  [unwired: 1 in, 3 out]
          n818 = call <vilib>:"ListHeaders.vi"("client handle"=w2243, "error in (no error)"=w2231) -> ("client handle out"=w2242:T6, "headers"=w2241:string, "error out"=w2236:errorcluster)  [unwired: 11 in]
          n819 = Greater Than 0?(x=w2238) -> (x > 0?=w2235:bool)
          n820 = Equal?(x=w2229, y=w2226) -> (x = y?=w2228:bool)
          n821 = Compound Arithmetic op=AND ("Mehrfacharithmetik")(invert w2236, w2235, w2228) -> (w2234:bool)
        }
        frame "Health check: Health check" {
          n822 = Concatenate Strings(w2261, "/healthcheck" ("String")) -> (w2254:string)
          n823 = call <vilib>:"GET.vi"("client handle"=w2265, "url"=w2254, "error in (no error)"=w2267) -> ("client handle out"=w2264:T6, "headers"=w2258:string, "body"=w2251:string, "error out"=w2253:errorcluster)  [unwired: 9 in]
          n824 = Match Pattern(string=w2258, regular expression="200" ("Regulärer Ausdruck")) -> (offset past match=w2259:i32)  [unwired: 1 in, 3 out]
          n825 = xnode "Regulären Ausdruck suchen"("Eingangs-String"=w2251, "Regulärer Ausdruck"="OK", "Schreibweise ignorieren (F)"=TRUE) -> ("Offset nach Übereinstimmung"=w2249:i32)  [unwired: 3 in, 4 out]
          n826 = call <vilib>:"ListHeaders.vi"("client handle"=w2264, "error in (no error)"=w2253) -> ("client handle out"=w2263:T6, "headers"=w2262:string, "error out"=w2257:errorcluster)  [unwired: 11 in]
          n827 = Greater Than 0?(x=w2259) -> (x > 0?=w2256:bool)
          n828 = Greater Or Equal To 0?(x=w2249) -> (x >= 0?=w2248:bool)
          n829 = Compound Arithmetic op=AND ("Mehrfacharithmetik")(invert w2257, w2256, w2248) -> (w2255:bool)
        }
        frame "Deinitialize HTTPs" {
          w2391 = ""
          n830 = call <vilib>:"CloseHandle.vi"("client handle"=w2390, "error in (no error)"=w2394) -> ("error out"=w2388:errorcluster)  [unwired: 13 in]
          n831 = call "LabVIEW.FGV.Store_ID.vi"("Command"=enum16{"clear", "write", "read"}."clear", "error in (no error)"=w2388) -> ("error out"=w2387:errorcluster)  [unwired: 8 in, 5 out]
          n832 = Not(x=w2387) -> (.not. x?=w2389:bool)
        }
      }
      "-H" <- w9
      "API Token" <- w35
      "Body" <- w6
      "Header" <- w7
      "Successful?" <- w33
      "Test other steps" <- w22
      "Test other steps 2" <- w21
      "URL" <- w11
      "Request body" <- w10
      n833 = feedback-in #1(w35) -> ()
      n834 = feedback-in #2(w37) -> ()
      n835 = control-ref of="Command"() -> (w19:refnum<vi>)
      n836 = property class="Enum (strict)"(reference=w19, error in=w14) -> (reference out=w15:refnum<vi>, error out=w16:errorcluster, "Strings []"=w18:string[], "Value"=w17:T2)
      n837 = Index Array(array=w18, index=w17) -> (element=w8:string)
      "Command name" <- w8
      n838 = Close Reference(reference=w15, error in (no error)=w16) -> (error out=w4:errorcluster)
      n839 = Bundle By Name(cluster=T1 {"Name"="", "URL"="", "Request body"="", "-H"="", "Hearder"="", "Bpdy"=""} ("Result_Cluster"), "Name"=w8, "URL"=w11, "Request body"=w10, "-H"=w9, "Hearder"=w7, "Bpdy"=w6) -> (→"Result_Cluster":T1)
    }
    frame Error {
    }
  }
  "error out" <- w2
